vi "DialogCreateMethod.vi"(0 "ClassWriterNative":refnum<class "ClassWriterNative.lvclass">, 1 "ClassItemRefIn":refnum<vi>, 5 "error in (no error)":errorcluster) -> (14 "ClassWriterNative":refnum<class "ClassWriterNative.lvclass">, 15 "ClassItemRefOut":refnum<vi>, 16 "CreateMethodData":T3={"MethodName"="", "RelativeMethodPath"=path "", "MethodDescription"="", "Scope/Visibility"=enum."Use Parent Folder Scope", "MethodTemplateName"="", "IconOut"=[], "RelativeProjectClassPath"="", "OpenViAfterCreation"=FALSE, "DynamicDispatchVi"=FALSE, "ExtraCreateParameters"=variant, "MustOverride"=FALSE, "MustCallParent"=FALSE, "IconDetails"={"IconSize"=enum."1 c-term high", "ImageRows(32)"=32, "ConnectorPaneHeight"=[]}, "AF-Option"=variant, "TemplatePath"=path ""} {"IconOut" format="%x"}, 17 "Cancelled":bool, 19 "error out":errorcluster)   [LabVIEW 2020, in "ClassWriterNative.lvclass"]
uses:
  <resource>/Framework/Providers/Open_GDS/ClassProviders/Provider_LvNativeClass/ClassWriterNative_class/ClassWriterNative.lvclass
  <resource>/Framework/Providers/Open_GDS/ClassProviders/Common/LvIcon_class/GDSLvIcon_ColorControl.ctl
  <resource>/Framework/Providers/Open_GDS/ClassProviders/Provider_BaseClassInterface/CreateMethodData.ctl
  <resource>/Framework/Providers/Open_GDS/ClassProviders/Provider_EndevoGOOP300/GOOP300_SubVIs/GOOP300_MethodScopeType.ctl
  <resource>/Framework/Providers/Open_GDS/ClassProviders/Provider_LvNativeClass/ClassWriterNative_class/IconDetails.ctl
  <resource>/Framework/Providers/Open_GDS/ClassProviders/Provider_LvNativeClass/ClassWriterNative_class/IconSize.ctl
  <resource>/Framework/Providers/Open_GDS/ClassProviders/Common/LvClass_class/GDSLvClass_PlugIn.ctl
  <resource>/Framework/Providers/Open_GDS/ClassProviders/Common/LvClass_class/GDSLvClass_PlugInTypes.ctl
  <resource>/Framework/Providers/Open_GDS/ClassProviders/Provider_LvNativeClass/ClassWriterNative_class/MethodInfo.ctl
  <resource>/Framework/Providers/Open_GDS/ClassProviders/Provider_LvNativeClass/ClassWriterNative_class/MethodType.ctl
  <resource>/Framework/Providers/Open_GDS/ClassProviders/Provider_LvNativeClass/ClassWriterNative_class/MethodInfo_Option.ctl
  <vilib>/Utility/miscctls.llb/LVPoint32TypeDef.ctl
  <vilib>/picture/picture.llb/imagedata.ctl
  <resource>/Framework/Providers/Open_GDS/ClassProviders/Provider_BaseClassInterface/ClassWriter_class/TemplateSettings.ctl
  <vilib>/Utility/miscctls.llb/LVRectTypeDef.ctl
  <resource>/Framework/Providers/Open_GDS/ClassProviders/Provider_EndevoGOOP400/EndevoG4ProviderName.ctl
  <vilib>/event_ctls.llb/lveventtype.ctl
  <resource>/Framework/Providers/Open_GDS/ClassProviders/Common/IconEditor/private/GDSIconEditor_IconDialog_Input.vi
  <resource>/Framework/Providers/Open_GDS/ClassProviders/Common/LvIcon_class/subvis/GDSLvIcon_TextDataType.ctl
  <resource>/Framework/Providers/Open_GDS/ClassProviders/Common/LvIcon_class/GDSLvIcon_WordCompressionType.ctl
  <resource>/Framework/Providers/Open_GDS/ClassProviders/Common/LvIcon_class/GDSLvIcon_TextAlignment.ctl
  <vilib>/Utility/miscctls.llb/LVPositionTypeDef.ctl
  <vilib>/Utility/miscctls.llb/LVPointTypeDef.ctl
  d442fafc-3c31-4c15-9ed3-3a3a20f58e2f.vi
  76481c0e-b793-4274-9995-712af1244245.vi
  <vilib>/Utility/config.llb/Read Key (String).vi
  <vilib>/regexp/Match Regular Expression.xnode
  <resource>/Framework/Providers/Open_GDS/ClassProviders/Provider_BaseClassInterface/ClassWriter_class/ClassWriter.lvclass
  <vilib>/Utility/lvfile.llb/NI_FileType.lvlib
  <vilib>/Utility/config.llb/NI_LVConfig.lvlib
panel:
  in  "PropertyNodeMethodNaming":enum16{"Read/Write Naming", "Get/Set Naming"}(ring) caption="Naming"
  out "MethodTemplateImage":picture
  out "_MethodsLocationOverrideInfo":string=" \n\n" caption="The method's location is controlled by\nthe method you override."
  in  "ClearIcon":bool
  in  "_AddFolder":bool
  in  "Filter":string
  in  ".vim":bool
  out "ProductPicture":picture
  out "_IconPreview":picture caption="Icon Preview"
  in  "_AddMessageClass":bool
  in  "_MethodIcons":bool
  in  "_TextAlignment":u16(ring) caption="Text Alignment" items=["Center", "Left", "Right"]
  in  "_IconSize":u16(ring) caption="Icon Size" items=["Full", "1 c-term high", "2 c-term high", "3 c-term high"]
  in  "_MustCallParent":bool caption="Must Call Parent"
  in  "_MustOverride":bool caption="Must Override"
  out "_VisibilityAndLlocationGrouping":string caption="Visibility and location"
  out "_IconGrouping":string caption="Icon"
  in  "_MethodSignature":u16(ring) caption="Method signature" items=["No signature", "-", "Add signature"]
  in  "_ShowContextHelp":bool
  in  "Help":bool
  in  "_CreateOpenClass":bool
  in  "_MethodIconName":string caption="Body Text"
  in  "_BodyBk":T1 caption="Body Background"
  in  "_BodyText":T1 caption="Body text"
  in  "_FontCompression":enum16{"Auto", "On", "Off"}(ring) caption="Font Compression"
  in  "_CapitalOnly":bool=TRUE caption="Force Capital Letters"
  out "_DubMethodName":string caption="This method already exists in the class"
  out "_Loading":string caption="Loading..."
  in  "_OverrideMethods":i32(listbox) caption="Override Methods"
  in  "_MethodType":T2(radio) caption="Method Type"
  in  "_Property":string[](tree) caption="Data Fields/Attributes"
  in  "_DynamicDispatch":bool caption="Dynamic Dispatch"
  in  "_Visibility":T7(radio) caption="Visibility"
  in  "_MethodLocation":i32(listbox) caption="Method Location"
  in  "_MethodName":string caption="Property Name"
  in  "_Cancel":bool
  in  "_CreateMethod":bool
  in  "_MethodDescription":string caption="Method description"
  in  "_Method":i32[](listbox) caption="Method Template"
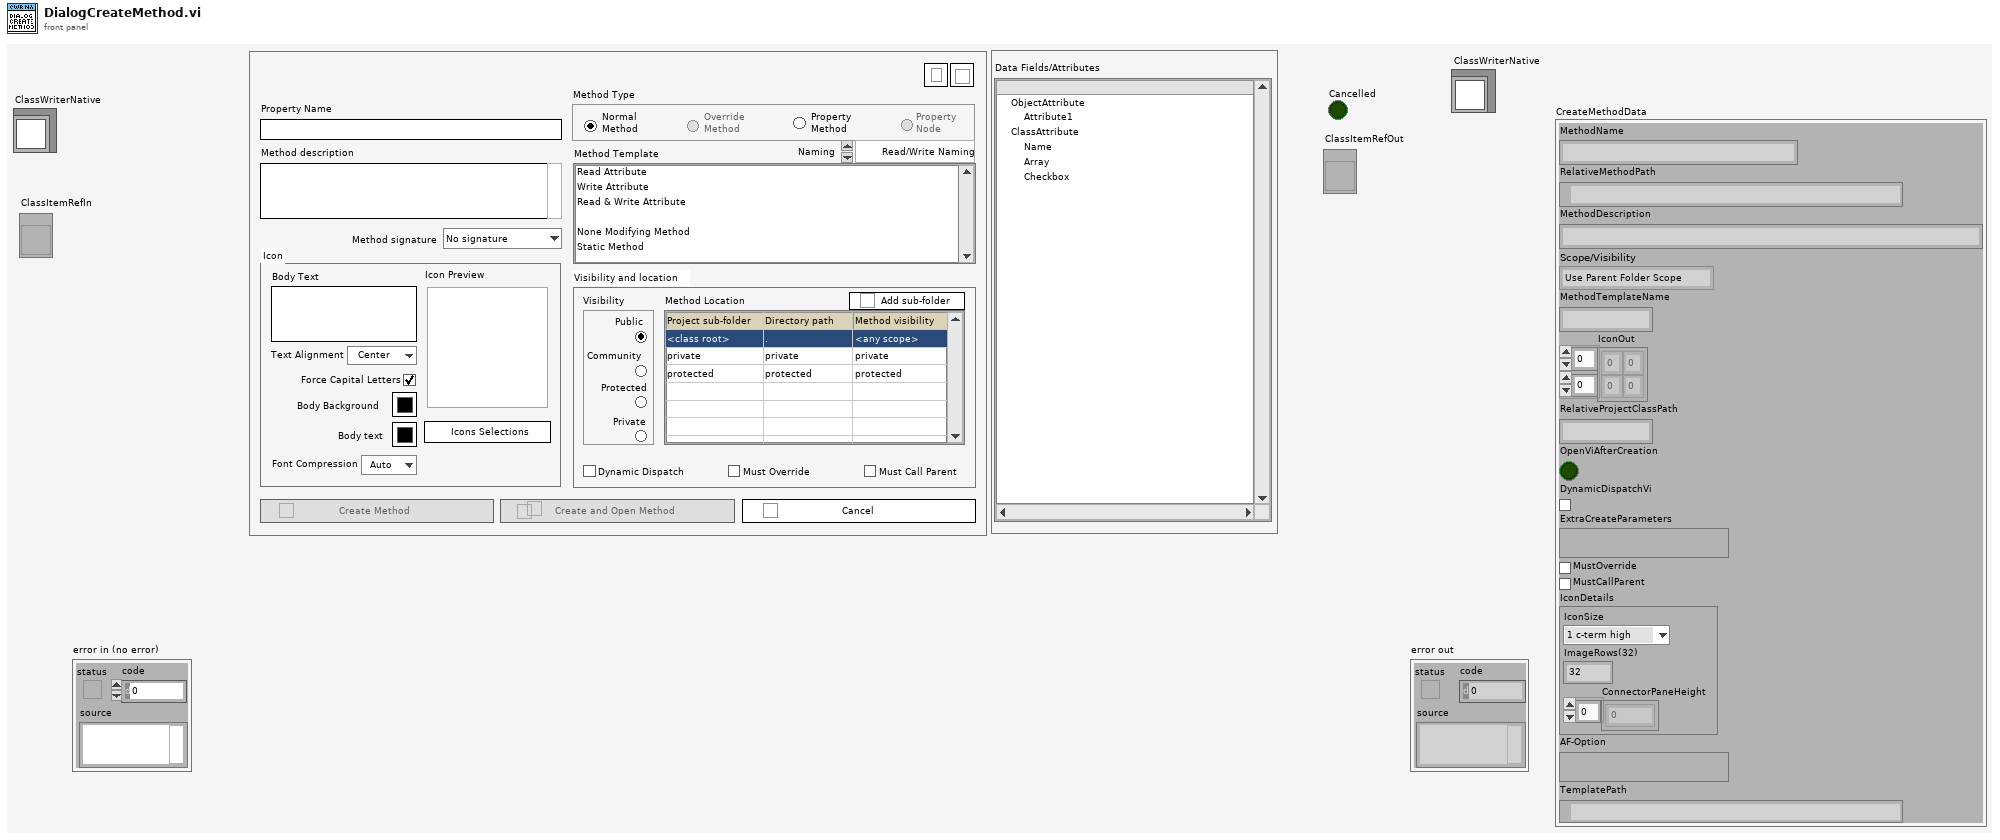
[diagram p1: front panel]
types:
  T1 = typedef "GDSLvIcon_ColorControl.ctl" = cluster{"Decal":bool, "Color":u32}
  T2 = enum32{"Normal Method", "Override Method", "Property Method", "Property Node"}
  T3 = typedef "ClassWriter.lvclass/CreateMethodData.ctl" = cluster{"MethodName":string, "RelativeMethodPath":path, "MethodDescription":string, "Scope/Visibility":T4, "MethodTemplateName":string, "IconOut":u8[][], "RelativeProjectClassPath":string, "OpenViAfterCreation":bool, "DynamicDispatchVi":bool, "ExtraCreateParameters":variant, "MustOverride":bool, "MustCallParent":bool, "IconDetails":T5, "AF-Option":variant, "TemplatePath":path}
  T4 = typedef "GOOP300_MethodScopeType.ctl" = enum16{"Use Parent Folder Scope", "Public", "Protected", "Private", "Community"}
  T5 = typedef "ClassWriterNative.lvclass/IconDetails.ctl" = cluster{"IconSize":T6, "ImageRows(32)":i32, "ConnectorPaneHeight":i32[]}
  T6 = typedef "ClassWriterNative.lvclass/IconSize.ctl" = enum16{"Full", "1 c-term high", "2 c-term high", "3 c-term high"}
  T7 = enum32{"Public", "Community", "Protected", "Private"}
  T8 = cluster{"Font Name":string, "Size":u16, "Bold":bool, "Italic":bool, "Underline":bool, "Strikeout":bool, "Color":u32}
  T9 = cluster{"AttributeNames":string[], "PropertyNode":bool, "FolderNames":string[]}
  T10 = typedef "GDSLvClass_PlugIn.ctl" = cluster{"Type":T11, "ID":string, "Version":string, "Path":path, "Name":string, "Data":variant}
  T11 = typedef "GDSLvClass_PlugInTypes.ctl" = enum16{"DesignPattern", "MethodTypes"}
  T12 = typedef "ClassWriterNative.lvclass/MethodInfo.ctl" = cluster{"Type":T13, "Name":string, "Path":path, "ExtraName":string, "Data":variant, "DynamicDispatch":T14}
  T13 = typedef "ClassWriterNative.lvclass/MethodType.ctl" = enum16{"Normal", "MethodPlugIn", "DesignPattern", "AF-Method"}
  T14 = typedef "ClassWriterNative.lvclass/MethodInfo_Option.ctl" = enum16{"Default", "OnAtStart", "OffAtStart", "AlwaysOn", "AlwaysOff"}
  T15 = typedef "LVPoint32TypeDef.ctl" = cluster{"Horizontal":i32, "Vertical":i32}
  T16 = typedef "imagedata.ctl" = cluster{"image type":i32, "image depth":i32, "image":u8[], "mask":u8[], "colors":u32[], "Rectangle":cluster{"left":i16, "top":i16, "right":i16, "bottom":i16}}
  T17 = typedef "ClassWriter.lvclass/TemplateSettings.ctl" = cluster{"CommonClassTemplate":bool, "DynamicDispatch":enum8{"False", "True", "Mixed"}, "MustOverride":enum8{"False", "True", "Mixed"}, "MustCallParent":enum8{"False", "True", "Mixed"}, "OnlyNormalMethod":bool, "OnlyPublic":bool}
  T18 = cluster{"Cancel":bool, "FolderNames":string[], "FolderPath":path[], "FolderType":enum32{"invalid scope", "public", "private", "protected", "community"}[], "ClassName":string, "ColorProtected":u32, "ColorPrivate":u32, "ColorPublic":u32, "Frame":u32, "Frame thickness":i32, "HeaderIcon":u8[][], "BodyIconHeight":i32, "BodyIconWidth":i32, "RelFolderPath":path[], "MethodIcon":u8[][], "OverRideLookUpDone":bool, "PropertyLookUpDone":bool, "AllOverrideMethods":path[], "ClassVIs":string[], "Open":bool, "OverrideScope":enum32{"invalid scope", "public", "private", "protected", "community"}[], "Signatures":cluster{"SignatureName":string[], "SignatureText":string[], "Current":i32}, "DesignPatterns":T10[], "NormalMethods":T12[], "OverrideMethods":T12[], "PropertyMethods":T12[], "MethodNames":string[], "ConnectorPaneHeight":i32[], "IconDetails":T5, "Offset":cluster{"X":i32, "Y":i32}, "OldOffset":cluster{"X":i32, "Y":i32}, "TextBounds":cluster{"FirstRow":i32, "FirstColumn":i32, "LastRow":i32, "LastColumn":i32}, "DraggingText":bool, "StartTextDraggingPos":T15, "Folders":path[], "IconPaths":cluster{i32, "path out":path}[], "Icons":T16[], "IconNames":string[], "DraggingIcon":bool, "StartTextDraggingPos 2":T15, "BgIconOffset":cluster{"X":i32, "Y":i32}, "Offset 2":cluster{"X":i32, "Y":i32}, "OldOffset 2":cluster{"X":i32, "Y":i32}, "CurrentIcon":cluster{"BgIcon":u8[][], "BgIconOffset":cluster{"X":i32, "Y":i32}, "BgIconMask":u8[], "ColorsOkayforiconToBeOnTopOf":u8[]}, "BgIconMask":u8[], "BodyIcon":u8[][], "BgIcon":u8[][], "HeaderBkColor":u32, "IconOut":u8[][], "IconSelected":i32, "IconDropped":i32, "Moving":bool, "IconPos":cluster{"left":i16, "top":i16, "right":i16, "bottom":i16}[], "BodyIconOut":u8[][], "AF":bool, "ActorVersion":string, "AF-MethodNames":string[], "AF-Methods":cluster{T12[]}[], "AF-Method":i32, "PropertyNodeMethods":T12[], "MethodLocation":string[][], "MethodCaptionName":string, "IsAPropertyDefinitionVI":bool[], "TemplateSettings":T17, "OverrideMethod":path, "Interface":bool, "RowStart(0)":i32, "ImageRows(32)":i32, "MethodVIs":path[], "MethodItemNames":string[], "OverrideMethodsNames":string[], "OverrideMethodsIdx":i32[], "Methods.DynamicDispatch":T14[], "Splitter0px":bool}
  T19 = enum8{"Enabled", "Disabled", "Disabled and Grayed Out"}
  T20 = enum16{"Full", "1 c-term high", "2 c-term high", "3 c-term high", "Off"}
  T21 = typedef "EndevoG4ProviderName.ctl" = enum16{"EndevoGOOP400"}
  T22 = enum32{"invalid scope", "public", "private", "protected", "community"}
  T23 = typedef "LVRectTypeDef.ctl" = cluster{"Left":i16, "Top":i16, "Right":i16, "Bottom":i16}
  T24 = typedef "lveventtype.ctl" = enum32{"Null", "Timeout", "Annotation Menu Selection", "Annotation Menu Selection?", "App Instance Close", "App Instance Close?", "Autoscale Range Change", "Bookmark Info Change", "Cell Edit", "Cell Edit?", "Cursor Grab", "Cursor Grab?", "Cursor Menu Selection", "Cursor Menu Selection?", "Cursor Move", "Cursor Release", "Data Change", "Direction Change", "Display State Change", "Drag Ended", "Drag Enter", "Drag Leave", "Drag Over", "Drag Source Update", "Drag Starting", "Drag Starting?", "Drop", "Exec State Change", "Key Down", "Key Down?", "Key Repeat", "Key Repeat?", "Key Up", "Listbox Double Click", "Menu Activation?", "Menu Selection (App)", "Menu Selection? (App)", "Menu Selection (User)", "Mouse Down", "Mouse Down?", "Mouse Enter", "Mouse Leave", "Mouse Move", "Mouse Up", "Mouse Wheel", "NI Security User Change (App)", "Pane Size", "Panel Close", "Panel Close?", "Panel Resize", "Plot Attribute Change", "Scale Range Change", "Shortcut Menu Activation?", "Shortcut Menu Selection (App)", "Shortcut Menu Selection? (App)", "Shortcut Menu Selection (User)", "Tree Double Click", "Tree Drag", "Tree Drag?", "Tree Drop", "Tree Drop?", "Tree Item Close", "Tree Item Close?", "Tree Item Open", "Tree Item Open?", "User Event", "Value Change"}
  T25 = typedef "GDSIconEditor_IconDialog_Input.vi" = cluster{"HeaderIcon":u8[][], "RowStart(0)":i32, "ImageRows(32)":i32, "FrameThickness(1)":u32, "FrameColor":u32, "IconTextDataType":T26, "BodyTextColor":u32, "BodyBackgroundColor":u32, "BodyIconHeight":i32, "BodyIconWidth":i32, "HeaderBackgroundColor":u32, "BodyIcon":u8[][], "Offset":cluster{"X":i32, "Y":i32}, "CurrentIcon":cluster{"BgIcon":u8[][], "BgIconOffset":cluster{"X":i32, "Y":i32}, "BgIconMask":u8[], "ColorsOkayforiconToBeOnTopOf":u8[]}}
  T26 = typedef "GDSLvIcon_TextDataType.ctl" = cluster{"Text":string, "Allow Only Capital Chars":bool, "Compression":T27, "Alignment":T28}
  T27 = typedef "GDSLvIcon_WordCompressionType.ctl" = enum16{"Auto", "On", "Off"}
  T28 = typedef "GDSLvIcon_TextAlignment.ctl" = enum16{"Center", "Left", "Right"}
  T29 = cluster{"BgIcon":u8[][], "BgIconOffset":cluster{"X":i32, "Y":i32}, "BgIconMask":u8[], "ColorsOkayforiconToBeOnTopOf":u8[]}
  T30 = typedef "LVPositionTypeDef.ctl" = cluster{"Left":i32, "Top":i32}
  T31 = typedef "LVPointTypeDef.ctl" = cluster{"Horizontal":i16, "Vertical":i16}
  T32 = typedef "GOOP400_Options.ctl" = cluster{"FlatFolderStructure":bool}
  T33 = enum32{"invalid scope", "public", "private", "protected", "community"}[]
  T34 = typedef "BaseProvider_IniFileSettings.ctl" = cluster{"ClassFolderSuffix":string, "InterfaceFolderSuffix":string, "InterfaceIcon":string, "FileNamingOption":T35, "DynamicDispatchStartValue":bool, "UseGetSetForPropertyNodeMethods":bool}
  T35 = typedef "BaseProvider_FileNamingOption.ctl" = enum16{"CamelCase", "Space", "Underscore"}
  T36 = cluster{"Major":u16, "Minor":u16, "Fix":u16, "Build":u16}
  T37 = typedef "AF_ClassType.ctl" = enum16{"NA", "Actor", "Message"}
  T38 = typedef "GDSLvClass_IconSettingsType.ctl" = cluster{"Frame":u32, "Frame thickness":u8, "Header Background":u32, "Header Text":u32, "ColorPublic":u32, "ColorProtected":u32, "ColorPrivate":u32, "Body Text":u32, "ClassBodyIcon":string}
  T39 = cluster{"SignatureName":string[], "SignatureText":string[], "Current":i32}
  T40 = typedef "eventvkey.ctl" = enum16{"ASCII", "Enter", "Return", "Shift", "Ctrl", "Alt", "Cmd", "Opt", "Caps", "NumLock", "Clear", "Break", "Up", "Down", "Left", "Right", "Insert", "Delete", "Home", "End", "PageUp", "PageDown", "Escape", "Help", "Pause", "ScrollLock", "F1", "F2", "F3", "F4", "F5", "F6", "F7", "F8", "F9", "F10", "F11", "F12", "F13", "F14", "F15", "F16", "F17", "F18", "F19", "F20", "F21", "F22", "F23", "F24", "Play", "VolumeUp", "VolumeDown", "Mute", "Two Byte Char"}
  T41 = typedef "LVMouseTypeDef.ctl" = cluster{"Mouse Position":cluster{"X":i32, "Y":i32}, "Mouse Modifiers":cluster{"Button Down":bool, "Shift Mod":bool, "Menu Mod":bool, "Option Mod":bool}}
  T42 = cluster{"FirstRow":i32, "FirstColumn":i32, "LastRow":i32, "LastColumn":i32}
  T43 = typedef "ColorControl.ctl" = cluster{"Decal":bool, "Color":u32}
  T44 = typedef "LVBoundsTypeDef.ctl" = cluster{"Width":u32, "Height":u32}
  T45 = cluster{"left":i16, "top":i16, "right":i16, "bottom":i16}
  T46 = typedef "NI_LVConfig.lvlib/Config Data RefNum.ctl" = refnum<k1>
  T47 = cluster{"PlugInName":string, "MethodSelected":string}
  T48 = cluster{"SignatureName":string[], "SignatureText":string[], i32}
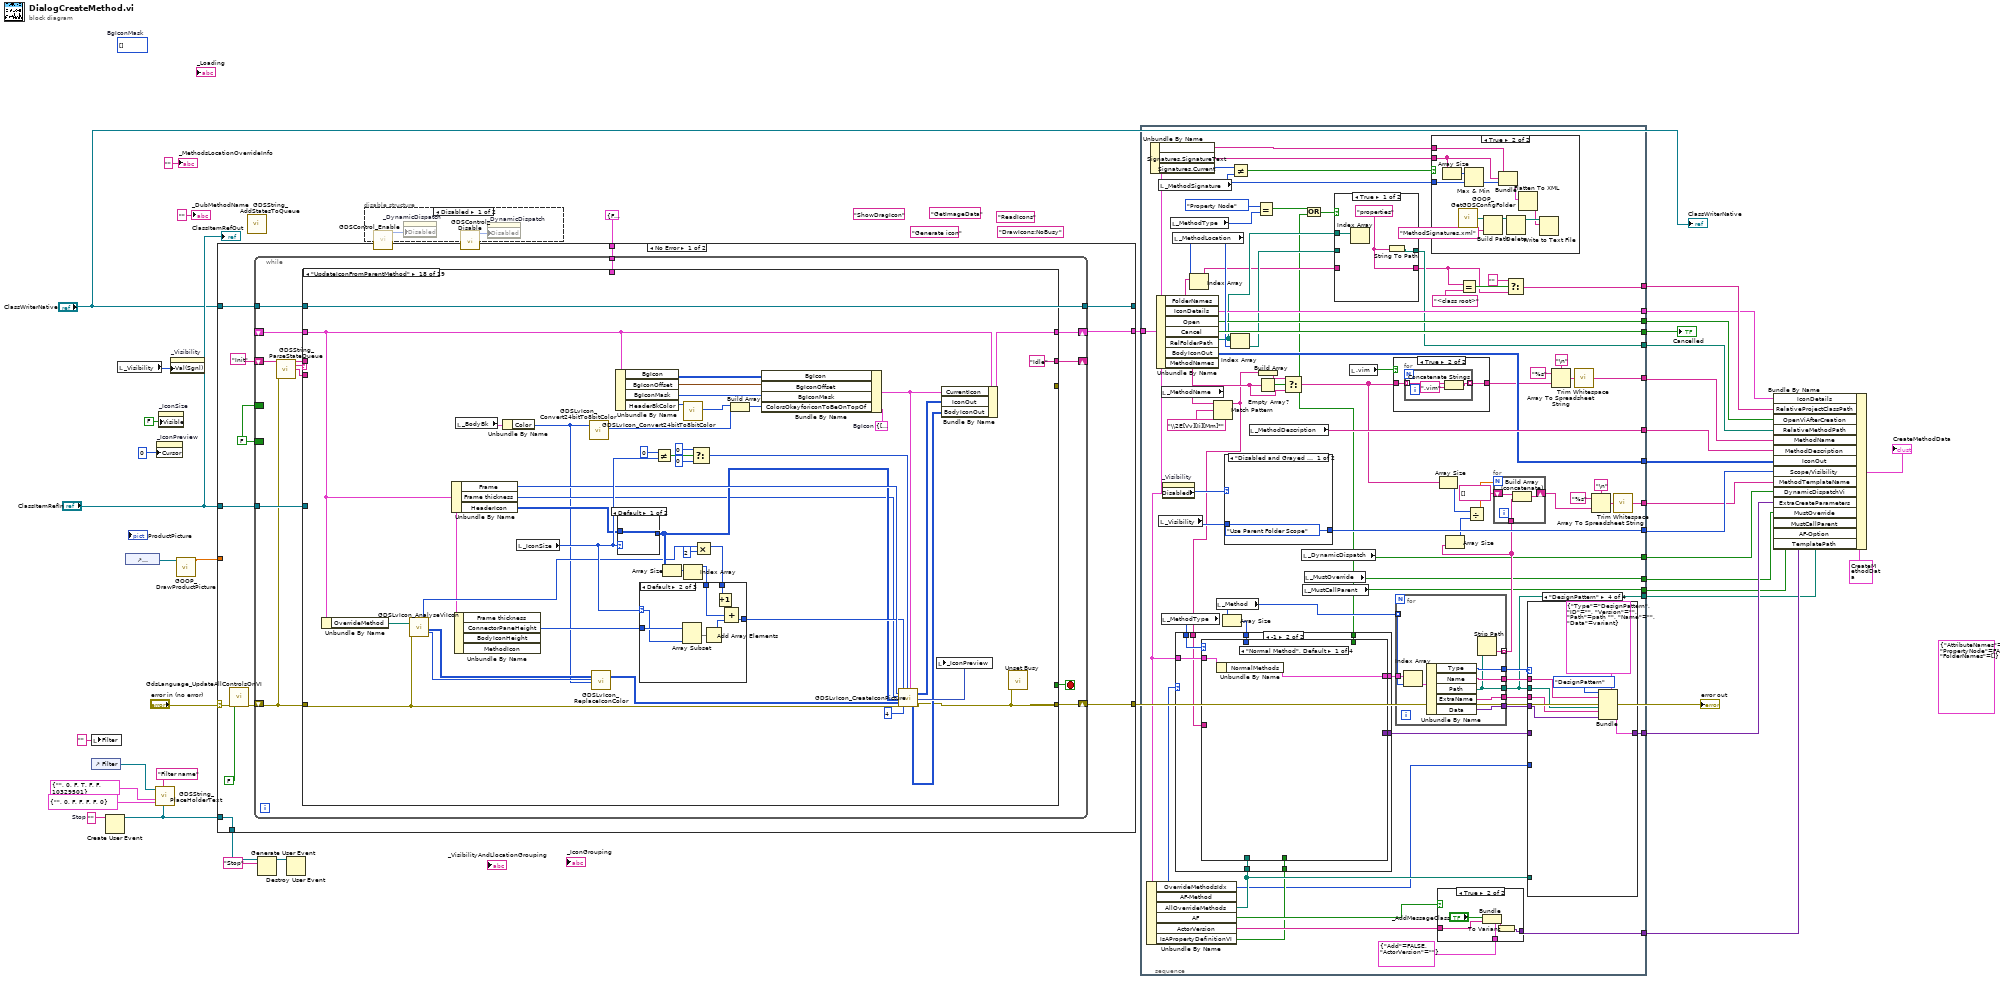
[diagram p0: block diagram]
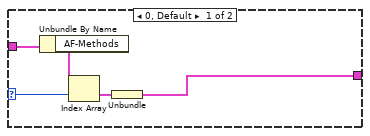
[diagram p5: hidden frame]
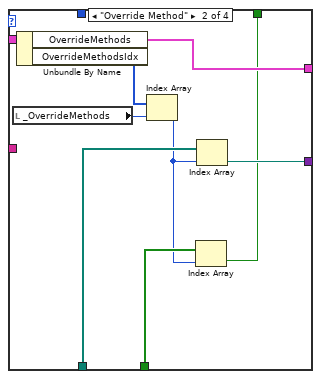
[diagram p6: hidden frame]
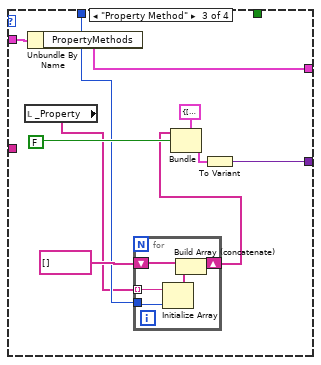
[diagram p7: hidden frame]
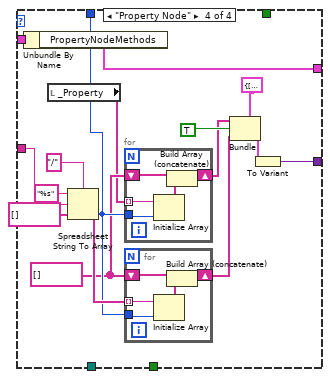
[diagram p8: hidden frame]
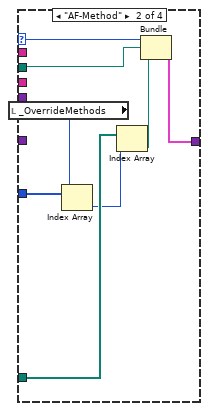
[diagram p11: hidden frame]
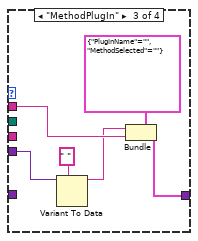
[diagram p12: hidden frame]
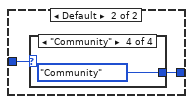
[diagram p14: hidden frame]
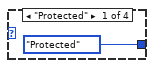
[diagram p15: hidden frame]
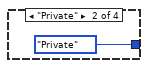
[diagram p16: hidden frame]
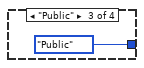
[diagram p17: hidden frame]
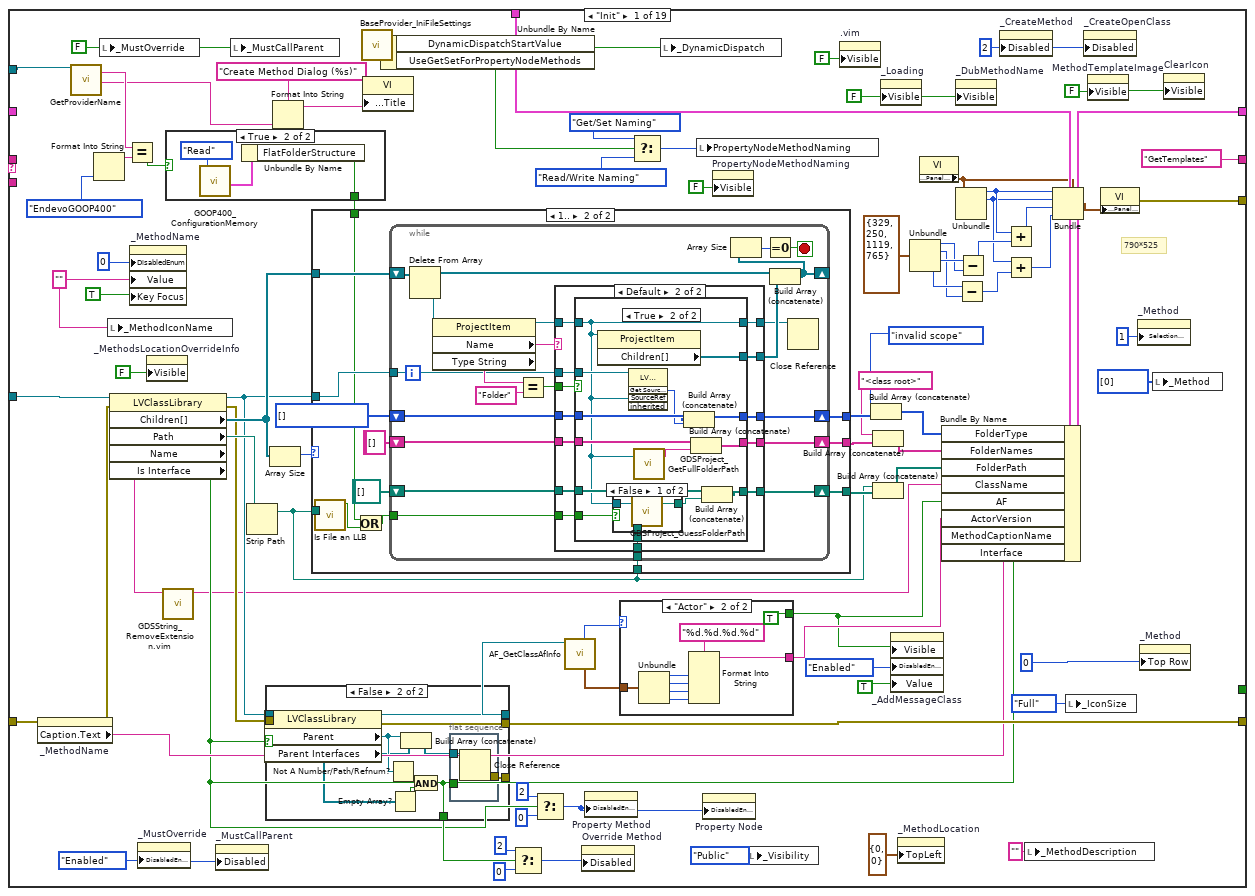
[diagram p18: hidden frame]
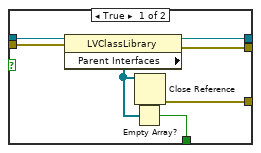
[diagram p20: hidden frame]
diagram:
  (unwired) "Generate icon"
  (unwired) "ShowDragIcon" ("t")
  (unwired) "GetImageData" ("y")
  (unwired) "DrawIcons:NoBusy" ("y")
  (unwired) "ReadIcons"
  w8 = ""  # Stop
  (unwired) T9 {"AttributeNames"=[], "PropertyNode"=FALSE, "FolderNames"=[]} ("cluster")
  (unwired) u8[] []  # BgIconMask
  n1 = control-ref of="Filter"() -> (w2:refnum<vi>)
  n2 = local write "Filter"("" ("Filter")) -> ()
  n3 = Create User Event(user event datatype=w8) -> (user event=w4:refnum<user-event>)  [unwired: 1 in, 1 out]
  n4 = local read "_Visibility"() -> (w11:T7)
  n5 = control-ref of="ProductPicture"() -> (w16:refnum<vi>)
  n6 = call <resource>:"GDSString_PlaceHolderText.vi"("BooleanUserEventToStopPlaceHolderVI"=w4, "PlaceholderText"="Filter name" ("InterfaceFilter"), "PlaceholderTextFont(Grey,Italic)"=T8 {"Font Name"="", "Size"=0, "Bold"=FALSE, "Italic"=TRUE, "Underline"=FALSE, "Strikeout"=FALSE, "Color"=10329501}, "NormalTextFont(Black)"=T8 {"Font Name"="", "Size"=0, "Bold"=FALSE, "Italic"=FALSE, "Underline"=FALSE, "Strikeout"=FALSE, "Color"=0}, "PlaceholderStringRef"=w2) -> ()  [unwired: 6 in, 1 out]
  n7 = property on="_IconPreview" class="Pict"("Cursor"=0) -> ()  [unwired: 2 in, 2 out]
  n8 = property on="_IconSize" class="Ring (strict)"("Visible"=FALSE) -> ()  [unwired: 2 in, 2 out]
  n9 = property on="_Visibility" class="RadioBtnsControl (strict)"("Val(Sgnl)"=w11) -> ()  [unwired: 2 in, 2 out]
  n10 = call <resource>:"GOOP_DrawProductPicture.vi"("ProductPictureControl"=w16) -> ("Zoom Factor"=w15:sgl)  [unwired: 10 in]
  n11 = case shown="No Error" "error in (no error)" {
    selector: "error in (no error)" -> [w47 w2528]
    tunnel: "ClassWriterNative" -> [w51 w2527]
    tunnel: [w53 w2528] -> w27
    tunnel: [w52 w2527] -> _
    tunnel: T18 {"Cancel"=FALSE, "FolderNames"=[], "FolderPath"=[], "FolderType"=[], "ClassName"="", "ColorProtected"=16777215, "ColorPrivate"=16777215, "ColorPublic"=16121600, "Frame"=0, "Frame thickness"=3, "HeaderIcon"=[], "BodyIconHeight"=0, "BodyIconWidth"=0, "RelFolderPath"=[], "MethodIcon"=[], "OverRideLookUpDone"=FALSE, "PropertyLookUpDone"=FALSE, "AllOverrideMethods"=[], "ClassVIs"=[], "Open"=FALSE, "OverrideScope"=[], "Signatures"={"SignatureName"=[], "SignatureText"=[], "Current"=-1}, "DesignPatterns"=[], "NormalMethods"=[], "OverrideMethods"=[], "PropertyMethods"=[], "MethodNames"=[], "ConnectorPaneHeight"=[], "IconDetails"={"IconSize"=enum."Full", "ImageRows(32)"=0, "ConnectorPaneHeight"=[]}, "Offset"={"X"=0, "Y"=0}, "OldOffset"={"X"=0, "Y"=0}, "TextBounds"={"FirstRow"=2, "FirstColumn"=1, "LastRow"=6, "LastColumn"=27}, "DraggingText"=FALSE, "StartTextDraggingPos"={"Horizontal"=0, "Vertical"=0}, "Folders"=[], "IconPaths"=[], "Icons"=[], "IconNames"=[], "DraggingIcon"=FALSE, "StartTextDraggingPos 2"={"Horizontal"=0, "Vertical"=0}, "BgIconOffset"={"X"=0, "Y"=0}, "Offset 2"={"X"=0, "Y"=0}, "OldOffset 2"={"X"=0, "Y"=0}, "CurrentIcon"={"BgIcon"=[], "BgIconOffset"={"X"=0, "Y"=0}, "BgIconMask"=[], "ColorsOkayforiconToBeOnTopOf"=[]}, "BgIconMask"=[], "BodyIcon"=[[0, 0, 0, 0, 0, 0, 0, 0, 0, 0, 255, 255, 0, 0, 255, 0, 0, 0, 255, 0, 0, 0, 0, 0, 0, 0, 0, 0, 0, 0], [0, 0, 0, 0, 0, 0, 0, 0, 0, 255, 0, 0, 255, 0, 255, 0, 0, 0, 255, 0, 0, 0, 0, 0, 0, 0, 0, 0, 0, 0], [0, 0, 0, 0, 0, 0, 0, 0, 0, 255, 255, 255, 255, 0, 255, 0, 0, 0, 255, 0, 0, 0, 0, 0, 0, 0, 0, 0, 0, 0], [0, 0, 0, 0, 0, 0, 0, 0, 0, 255, 0, 0, 255, 0, 255, 0, 0, 0, 255, 0, 0, 0, 0, 0, 0, 0, 0, 0, 0, 0], [0, 0, 0, 0, 0, 0, 0, 0, 0, 255, 0, 0, 255, 0, 255, 255, 255, 0, 255, 255, 255, 0, 0, 0, 0, 0, 0, 0, 0, 0], [0, 0, 255, 0, 0, 0, 255, 0, 0, 255, 255, 0, 0, 255, 0, 0, 255, 0, 255, 255, 0, 255, 255, 0, 0, 0, 255, 255, 0, 0], [0, 255, 0, 255, 0, 255, 0, 255, 0, 255, 0, 255, 0, 255, 255, 0, 255, 0, 255, 0, 0, 255, 0, 255, 0, 255, 0, 0, 0, 0], [0, 255, 0, 0, 0, 255, 0, 255, 0, 255, 255, 0, 0, 255, 0, 255, 255, 0, 255, 255, 0, 255, 255, 0, 0, 0, 255, 0, 0, 0], [0, 255, 0, 255, 0, 255, 0, 255, 0, 255, 0, 255, 0, 255, 0, 0, 255, 0, 255, 0, 0, 255, 0, 255, 0, 0, 0, 255, 0, 0], [0, 0, 255, 0, 0, 0, 255, 0, 0, 255, 0, 255, 0, 255, 0, 0, 255, 0, 255, 255, 0, 255, 0, 255, 0, 255, 255, 0, 0, 0], [0, 255, 0, 0, 0, 255, 0, 0, 255, 0, 0, 255, 0, 255, 0, 0, 255, 0, 255, 255, 0, 0, 255, 0, 0, 255, 255, 255, 0, 255], [255, 0, 255, 0, 255, 0, 255, 0, 255, 255, 0, 255, 0, 255, 255, 0, 255, 0, 255, 0, 0, 255, 0, 255, 0, 0, 255, 0, 0, 255], [255, 0, 0, 0, 255, 0, 255, 0, 255, 0, 255, 255, 0, 255, 0, 255, 255, 0, 255, 255, 0, 255, 0, 0, 0, 0, 255, 0, 0, 255], [255, 0, 255, 0, 255, 0, 255, 0, 255, 0, 0, 255, 0, 255, 0, 0, 255, 0, 255, 0, 0, 255, 0, 255, 0, 0, 255, 0, 0, 255], [0, 255, 0, 0, 0, 255, 0, 0, 255, 0, 0, 255, 0, 255, 0, 0, 255, 0, 255, 255, 0, 0, 255, 0, 0, 0, 255, 0, 0, 255], [0, 0, 0, 0, 0, 0, 0, 0, 0, 0, 0, 0, 0, 0, 255, 0, 0, 0, 0, 0, 0, 0, 0, 0, 0, 0, 0, 0, 0, 0], [0, 0, 0, 0, 0, 0, 0, 0, 0, 0, 0, 0, 0, 255, 0, 0, 0, 0, 0, 0, 0, 0, 0, 0, 0, 0, 0, 0, 0, 0], [0, 0, 0, 0, 0, 0, 0, 0, 0, 0, 0, 0, 0, 255, 255, 0, 0, 0, 0, 0, 0, 0, 0, 0, 0, 0, 0, 0, 0, 0], [0, 0, 0, 0, 0, 0, 0, 0, 0, 0, 0, 0, 0, 255, 0, 255, 0, 0, 0, 0, 0, 0, 0, 0, 0, 0, 0, 0, 0, 0], [0, 0, 0, 0, 0, 0, 0, 0, 0, 0, 0, 0, 0, 0, 255, 0, 0, 0, 0, 0, 0, 0, 0, 0, 0, 0, 0, 0, 0, 0], [0, 0, 0, 0, 0, 0, 0, 0, 0, 0, 0, 0, 0, 0, 0, 0, 0, 0, 0, 0, 0, 0, 0, 0, 0, 0, 0, 0, 0, 0], [0, 0, 0, 0, 0, 0, 0, 0, 0, 0, 0, 0, 0, 0, 0, 0, 0, 0, 0, 0, 0, 0, 0, 0, 0, 0, 0, 0, 0, 0]], "BgIcon"=[], "HeaderBkColor"=0, "IconOut"=[], "IconSelected"=0, "IconDropped"=-1, "Moving"=FALSE, "IconPos"=[], "BodyIconOut"=[], "AF"=TRUE, "ActorVersion"="", "AF-MethodNames"=[], "AF-Methods"=[], "AF-Method"=-1, "PropertyNodeMethods"=[], "MethodLocation"=[], "MethodCaptionName"=" ", "IsAPropertyDefinitionVI"=[], "TemplateSettings"={"CommonClassTemplate"=FALSE, "DynamicDispatch"=enum."False", "MustOverride"=enum."False", "MustCallParent"=enum."False", "OnlyNormalMethod"=FALSE, "OnlyPublic"=FALSE}, "OverrideMethod"=path "", "Interface"=TRUE, "RowStart(0)"=0, "ImageRows(32)"=32, "MethodVIs"=[], "MethodItemNames"=[], "OverrideMethodsNames"=[], "OverrideMethodsIdx"=[], "Methods.DynamicDispatch"=[], "Splitter0px"=FALSE} ("output cluster") -> [w50 _]
    tunnel: "ClassItemRefIn" -> [w49 _]
    tunnel: [w48 _] -> w39
    tunnel: w15 -> [_ _]
    tunnel: [w42 w2526] -> w5
    tunnel: w4 -> [w42 w2526]
    frame No Error {
      w43 = FALSE
      n12 = call <resource>:"GdsLanguage_UpdateAllControlsOnVI.vi"("error in (no error)"=w47, "CreateLanguageFile(Use this to create a languageFile)"=FALSE) -> ("error out"=w46:errorcluster)  [unwired: 16 in, 1 out]
      n13 = while {
        shift-right: [w65] -> w53
        shift-left: w46 -> [w56]
        shift-right: [w61] -> _
        shift-left: "Init" -> [w59]
        shift-right: [w66] -> w48
        shift-left: _ -> [w54]
        tunnel: w51 -> [w64]
        tunnel: [w64] -> w52
        tunnel: w50 -> [w63]
        tunnel: w49 -> [w62]
        border: w43 -> [_]
        border: w43 -> [_]
        stop <- w60 stop-if-true
        n14 = call <resource>:"GDSString_ParseStateQueue.vi"("State Queue"=w59, "Error In (no error)"=w56) -> ("Remaining States"=w57:string, "Current State"=w55:string, "Arguments"=w58:string)  [unwired: 9 in, 2 out]
        n15 = case shown="\"UpdateIconFromParentMethod\"" w55 {
          tunnel: w54 -> [_ w259 w342 w377 w396 w469 w502 w1663 w1741 w1787 w1798 w2111 w2156 w2177 w2196 w2300 w2414 w2467 w2521]
          tunnel: [w151 w293 w341 w376 w430 w466 w514 w1663 w1741 w1788 w1836 w2110 w2155 w2176 w2232 w2303 w2416 w2477 w2524] -> w66
          tunnel: w56 -> [w92 w290 w346 w370 w431 w476 w499 w1688 w1764 w1785 w1835 w2116 w2159 w2174 w2239 w2305 w2419 w2471 w2522]
          tunnel: [w98 w264 w346 w369 w390 w476 w500 w1688 w1764 w1785 w1834 w2109 w2150 w2174 w2240 w2305 w2418 w2463 w2522] -> w65
          tunnel: w64 -> [w114 w291 _ _ _ _ w498 _ _ _ _ _ w2152 _ _ _ _ _ _]
          tunnel: ["GetTemplates" w294 w337 "GetClassColors" "UpdateMethodSignatures" "UpdateIcon" w515 w1689 w1747 "Generate icon" "Exit" "Idle" "UpdateIcon" w2188 w2244 "Idle" "Idle" ("item tag") "Idle" ("item tag") "Exit"] -> w61
          tunnel: w63 -> [w149 _ _ _ _ _ _ _ _ _ _ _ _ _ _ _ _ _ _]
          tunnel: w62 -> [w150 w288 w350 w372 w400 _ w497 _ _ _ _ w2115 w2158 _ _ w2314 _ _ _]
          tunnel: [w86 _ _ _ _ _ _ _ _ _ _ _ _ _ _ _ _ _ _] -> _
          tunnel: [_ _ _ _ _ _ _ _ _ _ _ _ _ _ _ _ _ _ TRUE ("Cancel")] -> w60
          tunnel: w58 -> [_ _ _ _ _ _ _ _ _ _ _ _ _ _ _ _ _ _ _]
          tunnel: w57 -> [_ _ w336 _ _ _ _ w1689 w1747 _ _ _ _ w2188 _ _ _ _ _]
          frame "Init" {
            w78 = FALSE ("Visible")
            w89 = FALSE ("Dynamic dispatch")
            w109 = T19."Enabled" ("Disabled")
            w125 = FALSE ("Visible")
            w117 = u8 2 ("Disabled")
            w118 = "" ("Method Name")
            # "790*525"
            n16 = property on="_MethodName" class="Str"(error in=w92) -> (error out=w91:errorcluster, "Caption.Text"=w90:string)  [unwired: 1 in, 1 out]
            n17 = call-dynamic "GetProviderName.vi"("ClassWriterNative in"=w114) -> ("ProviderName"=w81:string, "TranslatedProviderName"=w79:string)  [unwired: 14 in, 3 out]
            n18 = Format Into String(EndevoG4ProviderName."EndevoGOOP400" ("ProviderName")) -> (resulting string=w105:string)  [unwired: 3 in, 1 out]
            n19 = local write "_MustOverride"(w89) -> ()
            n20 = local write "_MethodIconName"(w118) -> ()
            n21 = property class="LVClassLibrary"(reference=w150, error in=w91) -> (reference out=w124:refnum<vi>, error out=w123:errorcluster, "Children[]"=w147:refnum<vi>[], "Path"=w138:path, "Name"=w68:string, "Is Interface"=w83:bool)
            n22 = Equal?(x=w81, y=w105) -> (x = y?=w75:bool)
            n23 = property on="_MethodName" class="Str"("DisabledEnum"=u8 0 ("Disabled"), "Value"=w118, "Key Focus"=TRUE) -> ()  [unwired: 2 in, 2 out]
            n24 = property on="_MustOverride" class="Bool (strict)"("DisabledEnum"=w109) -> ()  [unwired: 2 in, 2 out]
            n25 = property on="_MethodsLocationOverrideInfo" class="Str"("Visible"=FALSE) -> ()  [unwired: 2 in, 2 out]
            n26 = call "GDSString_RemoveExtension.vim"("NameWithExtension"=w68) -> ("NameWithoutExtension"=w67:string)  [unwired: 9 in, 1 out]
            n27 = case shown="True" w75 {
              tunnel: [_ w153] -> w74
              frame False {
              }
              frame True {
                n28 = call <resource>:"GOOP400_ConfigurationMemory.vi"("Action"=enum16{"Read", "Load", "Save"}."Read") -> ("OptionsOut"=w154:T32)  [unwired: 17 in, 1 out]
                n29 = Unbundle By Name(w154) -> ("FlatFolderStructure"=w153:bool)
              }
            }
            n30 = property on="_MustCallParent" class="Bool (strict)"("Disabled"=w109) -> ()  [unwired: 2 in, 2 out]
            n31 = local write "_MustCallParent"(w89) -> ()
            n32 = Strip Path(path=w138) -> (stripped path=w110:path)  [unwired: 1 out]
            n33 = case shown="False" w83 {
              tunnel: w124 -> [w162 w173]
              tunnel: w123 -> [w161 w172]
              tunnel: [w159 w171] -> w98
              tunnel: [w158 w170] -> w97
              tunnel: [w157 w163] -> w87
              tunnel: [w156 w169] -> _
              frame True {
                n34 = property class="LVClassLibrary"(reference=w162, error in=w161) -> (reference out=w158:refnum<vi>, error out=w159:errorcluster, "Parent Interfaces"=w160:refnum<vi>[])
                n35 = Empty Array?(array=w160) -> (empty?=w157:bool)
                n36 = Close Reference(reference=w160) -> (error out=w156:errorcluster)  [unwired: 1 in]
              }
              frame False {
                n37 = property class="LVClassLibrary"(reference=w173, error in=w172) -> (reference out=w170:refnum<vi>, error out=w171:errorcluster, "Parent"=w167:refnum<vi>, "Parent Interfaces"=w166:refnum<vi>[])
                n38 = Not A Number/Path/Refnum?(number/path/refnum=w167) -> (NaN/Path/Refnum?=w165:bool)
                n39 = Empty Array?(array=w166) -> (empty?=w164:bool)
                n40 = Build Array (concatenate)(w167, w166) -> (w168:refnum<vi>[])
                n41 = And(x=w165, y=w164) -> (x .and. y?=w163:bool)
                n42 = flat-sequence {
                  tunnel: [w175] -> w169
                  tunnel: w168 -> [w174]
                  tunnel: w163 -> [_]
                  frame #0 {
                    n43 = Close Reference(reference=w174) -> (error out=w175:errorcluster)  [unwired: 1 in]
                  }
                }
              }
            }
            n44 = Array Size(array=w147) -> (size(s)=w146:i32)
            n45 = Format Into String(format string="Create Method Dialog (%s)", w79) -> (resulting string=w116:string)  [unwired: 2 in, 1 out]
            n46 = case shown="1.." w146 {
              tunnel: w147 -> [_ w196]
              tunnel: [_ w194] -> w144
              tunnel: [_ w193] -> w140
              tunnel: [_ w190] -> w142
              tunnel: w124 -> [_ w189]
              tunnel: w110 -> [_ w188]
              tunnel: w110 -> [_ w187]
              tunnel: w74 -> [_ w185]
              frame 0, Default {
              }
              frame 1.. {
                w191 = T33 [] items=["invalid scope", "public", "private", "protected", "community"]
                (unwired) path[] []
                (unwired) string[] []
                n47 = call <vilib>:"Is File an LLB.vi"("path"=w188) -> ("Is LLB?"=w186:bool)  [unwired: 9 in, 1 out]
                n48 = Or(x=w185, y=w186) -> (x .or. y?=w184:bool)
                n49 = while {
                  shift-right: [w199] -> _
                  shift-left: w196 -> [w218]
                  shift-right: [w208] -> w194
                  shift-left: path[] [] -> [w207]
                  shift-right: [w201] -> w193
                  shift-left: string[] [] -> [w204]
                  shift-right: [w202] -> w190
                  shift-left: w191 -> [w203]
                  tunnel: w189 -> [w200]
                  tunnel: w184 -> [w198]
                  tunnel: w187 -> [w197]
                  stop <- w215 stop-if-true
                  n50 = Delete From Array(array=w218) -> (deleted portion=w214:refnum<vi>, array with subset deleted=w217:refnum<vi>[])  [unwired: 2 in]
                  n51 = property class="ProjectItem"(reference=w214) -> (reference out=w210:refnum<vi>, "Name"=w205:string, "Type String"=w213:string)  [unwired: 1 in, 1 out]
                  n52 = Equal?(x=w213, y="Folder") -> (x = y?=w211:bool)
                  n53 = case shown="Default" w205 {
                    tunnel: w211 -> [_ w235]
                    tunnel: w210 -> [w221 w234]
                    tunnel: [_ w233] -> w209
                    tunnel: [w219 w226] -> w201
                    tunnel: [w222 w232] -> w208
                    tunnel: w207 -> [w222 w231]
                    tunnel: [w221 w230] -> w206
                    tunnel: w204 -> [w219 w229]
                    tunnel: w203 -> [w220 w228]
                    tunnel: [w220 w227] -> w202
                    tunnel: w200 -> [_ w225]
                    tunnel: w198 -> [_ w224]
                    tunnel: w197 -> [_ w223]
                    frame "Util", "Utils" {
                    }
                    frame Default {
                      n54 = case shown="True" w235 {
                        tunnel: w234 -> [w238 w243]
                        tunnel: [_ w253] -> w233
                        tunnel: [w236 w252] -> w226
                        tunnel: w231 -> [w239 w250]
                        tunnel: [w239 w251] -> w232
                        tunnel: [w238 w243] -> w230
                        tunnel: w229 -> [w236 w246]
                        tunnel: w228 -> [w237 w248]
                        tunnel: [w237 w247] -> w227
                        tunnel: w225 -> [_ w245]
                        tunnel: w224 -> [_ w241]
                        tunnel: w223 -> [_ w240]
                        frame False {
                        }
                        frame True {
                          n55 = property class="ProjectItem"(reference=w243) -> ("Children[]"=w253:refnum<vi>[])  [unwired: 1 in, 2 out]
                          n56 = case shown="False" w241 {
                            tunnel: [w255 w256] -> w249
                            tunnel: w243 -> [w254 _]
                            tunnel: w240 -> [_ w256]
                            frame False {
                              n57 = call <resource>:"GDSProject_GuessFolderPath.vi"("ProjectItem"=w254) -> ("Path"=w255:path)  [unwired: 15 in, 3 out]
                            }
                            frame True {
                            }
                          }
                          n58 = invoke class="LVClassLibrary" method="Get Source Scope"(reference=w245, "SourceRef"=w243) -> ("GetSourceScope"=w244:T22)  [unwired: 3 in, 4 out]
                          n59 = call <resource>:"GDSProject_GetFullFolderPath.vi"("Folder Item"=w243) -> ("ProjectClassPath"=w242:string)  [unwired: 17 in, 1 out]
                          n60 = Build Array (concatenate)(w248, w244) -> (w247:T33)
                          n61 = Build Array (concatenate)(w246, w242) -> (w252:string[])
                          n62 = Build Array (concatenate)(w250, w249) -> (w251:path[])
                        }
                      }
                    }
                  }
                  n63 = Build Array (concatenate)(w217, w209) -> (w199:refnum<vi>[])
                  n64 = Array Size(array=w199) -> (size(s)=w216:i32)
                  n65 = Equal To 0?(x=w216) -> (x = 0?=w215:bool)
                  n66 = Close Reference(reference=w206) -> ()  [unwired: 1 in, 1 out]
                }
              }
            }
            n67 = call <resource>:"BaseProvider_IniFileSettings.vi"() -> ("IniFileSettings"=w77:T34)  [unwired: 18 in, 1 out]
            n68 = property class="VI"("Front Panel.Title"=w116) -> ()  [unwired: 2 in, 2 out]
            n69 = Unbundle By Name(w77) -> ("DynamicDispatchStartValue"=w76:bool, "UseGetSetForPropertyNodeMethods"=w72:bool)
            n70 = Select(t=u8 2 ("Disabled"), s=w87, f=u8 0 ("Disabled")) -> (s? t:f=w122:u8)
            n71 = Select(t=u8 2 ("Disabled"), s=w83, f=u8 0 ("Disabled")) -> (s? t:f=w82:u8)
            n72 = call <resource>:"AF_GetClassAfInfo.vi"("DeriveFromClassRef"=w97) -> ("AF Library Version"=w96:T36, "ClassType"=w94:T37)  [unwired: 5 in, 4 out]
            n73 = property on="Override Method" class="Bool (strict)"("Disabled"=w122) -> ()  [unwired: 2 in, 2 out]
            n74 = property on="Property Method" class="Bool (strict)"("DisabledEnum"=w82) -> ()  [unwired: 2 in, 2 out]
            n75 = case shown="\"Actor\"" w94 {
              tunnel: w96 -> [_ w178]
              tunnel: [_ w177] -> w95
              tunnel: [_ TRUE ("LimitToSpecificProviderTypeOfSameType(True)")] -> w93
              frame "NA", Default {
              }
              frame "Actor" {
                n76 = Unbundle(w178) -> ("Major"=w182:u16, "Minor"=w181:u16, "Fix"=w180:u16, "Build"=w179:u16)
                n77 = Format Into String(format string="%d.%d.%d.%d", w182, w181, w180, w179) -> (resulting string=w177:string)  [unwired: 2 in, 1 out]
              }
            }
            n78 = Select(t=enum16{"Read/Write Naming", "Get/Set Naming"}."Get/Set Naming" ("PropertyNodeMethodNaming"), s=w72, f=enum16{"Read/Write Naming", "Get/Set Naming"}."Read/Write Naming" ("PropertyNodeMethodNaming")) -> (s? t:f=w71:enum16{"Read/Write Naming", "Get/Set Naming"})
            n79 = local write "_DynamicDispatch"(w76) -> ()
            n80 = local write "PropertyNodeMethodNaming"(w71) -> ()
            n81 = property on="Property Node" class="Bool (strict)"("DisabledEnum"=w82) -> ()  [unwired: 2 in, 2 out]
            n82 = property on="PropertyNodeMethodNaming" class="Enum (strict)"("Visible"=FALSE) -> ()  [unwired: 2 in, 2 out]
            n83 = local write "_Visibility"(T7."Public" ("_Visibility")) -> ()
            n84 = property on=".vim" class="Bool (strict)"("Visible"=FALSE) -> ()  [unwired: 2 in, 2 out]
            n85 = Build Array (concatenate)(T22."invalid scope" ("Source Scope:Get"), w142) -> (w141:T33)
            n86 = Build Array (concatenate)("<class root>" ("Name"), w140) -> (w145:string[])
            n87 = Build Array (concatenate)(w110, w144) -> (w143:path[])
            n88 = property on="_Loading" class="Str"("Visible"=w125) -> ()  [unwired: 2 in, 2 out]
            n89 = property on="_AddMessageClass" class="Bool (strict)"("Visible"=w93, "DisabledEnum"=T19."Enabled" ("Disabled"), "Value"=TRUE ("LimitToSpecificProviderTypeOfSameType(True)")) -> ()  [unwired: 2 in, 2 out]
            n90 = property on="_MethodLocation" class="MCListbox (strict)"("TopLeft"=cluster{"Row":u32, "Column":u32} {"Row"=0, "Column"=0} ("Top Left Visible Cell")) -> ()  [unwired: 2 in, 2 out]
            n91 = Unbundle(T23 {"Left"=329, "Top"=250, "Right"=1119, "Bottom"=765} ("Front Panel Window:Panel Bounds")) -> ("Left"=w136:i16, "Top"=w134:i16, "Right"=w137:i16, "Bottom"=w135:i16)
            n92 = property class="VI"() -> ("Front Panel.PanelBounds"=w131:T23)  [unwired: 2 in, 2 out]
            n93 = Bundle By Name(cluster=w149, "FolderType"=w141, "FolderNames"=w145, "FolderPath"=w143, "ClassName"=w67, "AF"=w93, "ActorVersion"=w95, "MethodCaptionName"=w90, "Interface"=w83) -> (w151:T18)
            n94 = property on="_DubMethodName" class="Str"("Visible"=w125) -> ()  [unwired: 2 in, 2 out]
            n95 = Unbundle(w131) -> ("Left"=w130:i16, "Top"=w129:i16)  [unwired: 2 out]
            n96 = Subtract(x=w135, y=w134) -> (x-y=w132:i16)
            n97 = Subtract(x=w137, y=w136) -> (x-y=w133:i16)
            n98 = property on="_CreateMethod" class="Bool"("Disabled"=w117) -> ()  [unwired: 2 in, 2 out]
            n99 = Add(x=w130, y=w133) -> (x+y=w128:i16)
            n100 = Add(x=w129, y=w132) -> (x+y=w127:i16)
            n101 = local write "_MethodDescription"("" ("Method description")) -> ()
            n102 = Bundle(cluster=w131, "Left"=w130, "Top"=w129, "Right"=w128, "Bottom"=w127) -> (w126:T23)
            n103 = local write "_IconSize"(T20."Full" ("_IconSize")) -> ()
            n104 = property on="_CreateOpenClass" class="Bool"("Disabled"=w117) -> ()  [unwired: 2 in, 2 out]
            n105 = property on="MethodTemplateImage" class="Pict"("Visible"=w78) -> ()  [unwired: 2 in, 2 out]
            n106 = property class="VI"("Front Panel.PanelBounds"=w126) -> (error out=w86:errorcluster)  [unwired: 2 in, 1 out]
            n107 = property on="_Method" class="LstBox (strict)"("Selection Mode"=1) -> ()  [unwired: 2 in, 2 out]
            n108 = property on="_Method" class="LstBox (strict)"("Top Row"=u8 0 ("Disabled")) -> ()  [unwired: 2 in, 2 out]
            n109 = local write "_Method"(i32[] [0] ("_Method")) -> ()
            n110 = property on="ClearIcon" class="Bool"("Visible"=w78) -> ()  [unwired: 2 in, 2 out]
          }
          frame "GetTemplates" {
            n111 = call <resource>:"GetAllMethodsTypesForClass.vi"("ClassWriterNative"=w291, "ClassItemRefIn"=w288, "error in"=w290) -> ("DesignPattern"=w289:T10[], "NormalMethods"=w284:T12[], "OverrideMethods"=w287:T12[], "PropertyMethods"=w286:T12[], "ConnectorPaneHeight"=w283:i32[], "TemplateSettings"=w280:T17, "PropertyNodeMethods"=w282:T12[], "error out"=w264:errorcluster)  [unwired: 4 in, 1 out]
            n112 = Unbundle By Name(w280) -> ("OnlyNormalMethod"=w279:bool, "DynamicDispatch"=w275:enum8{"False", "True", "Mixed"}, "MustOverride"=w268:enum8{"False", "True", "Mixed"}, "MustCallParent"=w267:enum8{"False", "True", "Mixed"}, "OnlyPublic"=w266:bool)
            n113 = case shown="False" w266 {
              tunnel: [w297 w298] -> w265
              tunnel: [T19."Enabled" ("Disabled") w298] -> w262
              frame False {
                n114 = property on="_MethodLocation" class="MCListbox (strict)"() -> ("DisabledEnum"=w297:T19)  [unwired: 2 in, 2 out]
              }
              frame True {
                w298 = T19."Disabled and Grayed Out" ("Disabled")
              }
            }
            n115 = Array Size(array=w282) -> (size(s)=w281:i32)
            n116 = case shown="False" w279 {
              tunnel: w281 -> [w320 _]
              tunnel: [w319 T19."Enabled" ("Disabled")] -> w278
              tunnel: [T19."Enabled" ("Disabled") T19."Disabled and Grayed Out" ("Disabled")] -> w277
              tunnel: [T2."Normal Method" ("_MethodType") T2."Normal Method" ("_MethodType")] -> w276
              frame False {
                n117 = case shown="0" w320 {
                  tunnel: [T19."Enabled" ("Disabled") T19."Disabled and Grayed Out" ("Disabled")] -> w319
                  frame Default {
                  }
                  frame 0 {
                  }
                }
              }
              frame True {
              }
            }
            n118 = property on="_MethodLocation" class="MCListbox (strict)"("DisabledEnum"=w265) -> ()  [unwired: 2 in, 2 out]
            n119 = property on="_Visibility" class="RadioBtnsControl (strict)"("Disabled"=w262, "Value"=T7."Public" ("_Visibility")) -> ()  [unwired: 2 in, 2 out]
            n120 = for {
              tunnel: w284 -> [w329] mode=indexing
              tunnel: [w330] -> w285 mode=indexing
              tunnel: [w328] -> w260 mode=indexing
              tunnel: [w327] -> w261 mode=indexing
              tunnel: [w326] -> w257 mode=indexing
              n121 = Unbundle(w329) -> ("Name"=w328:string, "Path"=w327:path, "DynamicDispatch"=w326:T14)  [unwired: 3 out]
              n122 = case shown="\"\"" w328 {
                tunnel: [0 -1] -> w330
                frame Default {
                }
                frame "" {
                }
              }
            }
            n123 = case shown="\"Mixed\"" w275 {
              tunnel: [T19."Enabled" ("Disabled") T19."Disabled and Grayed Out" ("Disabled") T19."Disabled and Grayed Out" ("Disabled")] -> w274
              tunnel: [TRUE TRUE FALSE] -> w273
              frame "Mixed" {
              }
              frame "True" {
              }
              frame "False" {
              }
            }
            n124 = case shown="\"Mixed\"" w268 {
              tunnel: [T19."Enabled" ("Disabled") T19."Disabled and Grayed Out" ("Disabled") T19."Disabled and Grayed Out" ("Disabled")] -> w271
              tunnel: [FALSE TRUE FALSE] -> w272
              frame "Mixed" {
              }
              frame "True" {
              }
              frame "False" {
              }
            }
            n125 = case shown="\"Mixed\"" w267 {
              tunnel: [T19."Enabled" ("Disabled") T19."Disabled and Grayed Out" ("Disabled") T19."Disabled and Grayed Out" ("Disabled")] -> w270
              tunnel: [FALSE TRUE FALSE] -> w269
              frame "Mixed" {
              }
              frame "True" {
              }
              frame "False" {
              }
            }
            n126 = property on="_Method" class="LstBox (strict)"("Item Names"=w260, "Item Symbols"=w285) -> ()  [unwired: 2 in, 2 out]
            n127 = Bundle By Name(cluster=w259, "DesignPatterns"=w289, "NormalMethods"=w284, "OverrideMethods"=w287, "PropertyMethods"=w286, "MethodVIs"=w261, "MethodItemNames"=w260, "ConnectorPaneHeight"=w283, "PropertyNodeMethods"=w282, "TemplateSettings"=w280, "Methods.DynamicDispatch"=w257) -> (w293:T18)
            n128 = Array Size(array=w284) -> (size(s)=w292:i32)
            n129 = property on="_MethodType" class="RadioBtnsControl (strict)"("DisabledEnum"=w277, "Value"=w276) -> ()  [unwired: 2 in, 2 out]
            n130 = property on="_DynamicDispatch" class="Bool (strict)"("Disabled"=w274, "Value"=w273) -> ()  [unwired: 2 in, 2 out]
            n131 = property on="_MustOverride" class="Bool (strict)"("Disabled"=w271, "Value"=w272) -> ()  [unwired: 2 in, 2 out]
            n132 = property on="_MustCallParent" class="Bool (strict)"("Disabled"=w270, "Value"=w269) -> ()  [unwired: 2 in, 2 out]
            n133 = Unbundle By Name(w259) -> ("Interface"=w258:bool)
            n134 = case shown="1.." w292 {
              tunnel: ["Exit" "UpdateScopeList"] -> w294
              frame 0, Default {
                n135 = One Button Dialog(message="No method templates where found for this class" ("format string")) -> ()  [unwired: 1 in, 1 out]
              }
              frame 1.. {
              }
            }
            n136 = case shown="False" w258 {
              tunnel: w278 -> [w295 _]
              frame False {
                n137 = property on="Property Node" class="Bool (strict)"("DisabledEnum"=w295) -> ()  [unwired: 2 in, 2 out]
              }
              frame True {
              }
            }
          }
          frame "UpdateScopeList" {
            n138 = property class="LVClassLibrary"(reference=w350) -> ("Path"=w345:path)  [unwired: 1 in, 2 out]
            n139 = Unbundle By Name(w342) -> ("FolderNames"=w348:string[], "FolderPath"=w349:path[], "FolderType"=w347:T33)
            n140 = Strip Path(path=w345) -> (stripped path=w344:path)  [unwired: 1 out]
            n141 = for {
              tunnel: w349 -> [w365] mode=indexing
              tunnel: w344 -> [w364]
              tunnel: w348 -> [w351] mode=indexing
              tunnel: w347 -> [w355] mode=indexing
              tunnel: [w357] -> w339 mode=indexing
              tunnel: [w352] -> w340 mode=indexing
              n142 = Path To String(path=w364) -> (string=w362:string)
              n143 = Path To String(path=w365) -> (string=w363:string)
              n144 = Search and Replace String(input string=w363, search string=w362) -> (result string=w361:string)  [unwired: 6 in, 3 out]
              n145 = case shown="Default" w355 {
                selector: w355 -> [_ w368]
                tunnel: ["<any scope>" w367] -> w354
                frame "invalid scope" {
                }
                frame Default {
                  n146 = Format Into String(w368) -> (resulting string=w367:string)  [unwired: 3 in, 1 out]
                }
              }
              n147 = String Subset(string=w361, offset (0)=1) -> (substring=w353:string)  [unwired: 1 in]
              n148 = String To Path(string=w353) -> (path=w352:path)
              n149 = Empty String/Path?(string/path=w353) -> (empty?=w359:bool)
              n150 = Select(t=".", s=w359, f=w353) -> (s? t:f=w356:string)
              n151 = Build Array(w351, w356, w354) -> (w357:string[])
            }
            n152 = Bundle By Name(cluster=w342, "RelFolderPath"=w340, "MethodLocation"=w339) -> (w341:T18)
            n153 = property on="_MethodLocation" class="MCListbox (strict)"("ItemNames"=w339, "Value"=0 ("Method Location")) -> ()  [unwired: 2 in, 2 out]
            n154 = call <resource>:"GDSString_AddStatesToQueue.vi"("EmptyQueueNextState"="GetCurrentClassMethods", "State(s) in (\"\")"=w336) -> ("States Out"=w337:string)  [unwired: 13 in]
          }
          frame "GetCurrentClassMethods" {
            n155 = invoke class="LVClassLibrary" method="Get All Descendents"(reference=w372, error in=w370, "Type"="VI") -> (error out=w369:errorcluster, "All Descendents"=w373:refnum<vi>[])  [unwired: 4 in, 5 out]
            n156 = for {
              tunnel: w373 -> [w387] mode=indexing
              tunnel: [w379] -> w371 mode=indexing
              n157 = property class="ProjectItem"(reference=w387) -> (reference out=w382:refnum<vi>, error out=w384:errorcluster, "Reference"=w381:refnum<vi>)  [unwired: 1 in]
              n158 = property class="VI"(reference=w381, error in=w384) -> (reference out=w385:refnum<vi>, error out=w386:errorcluster, "Name"=w380:string)
              n159 = Close Reference(reference=w385, error in (no error)=w386) -> (error out=w383:errorcluster)
              n160 = Close Reference(reference=w382, error in (no error)=w383) -> ()  [unwired: 1 out]
              n161 = Match Pattern(string=w380, regular expression=":") -> (after substring=w379:string)  [unwired: 1 in, 3 out]
            }
            n162 = Bundle By Name(cluster=w377, "ClassVIs"=w371) -> (w376:T18)
          }
          frame "GetClassColors" {
            w421 = u8 32 ("x")
            n163 = Unbundle By Name(w396) -> ("Interface"=w395:bool)
            n164 = call <resource>:"GDSLvClass_ReadClassColors.vi"("Library Refnum"=w400, "error in (no error)"=w431) -> ("LvClassIconSettings"=w412:T38, "error out"=w422:errorcluster)  [unwired: 12 in, 4 out]
            n165 = Unbundle By Name(w412) -> ("ColorProtected"=w409:u32, "ColorPrivate"=w410:u32, "ColorPublic"=w405:u32, "Frame"=w411:u32, "Frame thickness"=w408:u8, "Body Text"=w407:u32)
            n166 = case shown="True" w395 {
              tunnel: w422 -> [w432 w444]
              tunnel: w400 -> [w433 w443]
              tunnel: [w433 w442] -> w397
              tunnel: [_ w440] -> w394
              tunnel: [_ w439] -> w393
              tunnel: [_ w438] -> w392
              tunnel: [w432 w435] -> w391
              tunnel: [_ w434] -> w389
              frame True {
              }
              frame False {
                n167 = property class="LVClassLibrary"(reference=w443, error in=w444) -> (reference out=w442:refnum<vi>, error out=w441:errorcluster, "Member Data"=w437:refnum<vi>)
                n168 = call <resource>:"GDSLvIcon_AnalyseViIcon.vi"("ViRef/LvCLassRef/LvLibRef/ViPath/2D_Image"=w437, "error in (no error)"=w441) -> ("Splitter0px"=w434:bool, "ValidHeaderIcon"=w440:bool, "HeaderIcon"=w439:u8[][], "HeaderBkColor"=w438:u32, "error out"=w436:errorcluster)  [unwired: 4 in, 9 out]
                n169 = Close Reference(reference=w437, error in (no error)=w436) -> (error out=w435:errorcluster)
              }
            }
            n170 = Equal?(x=w405, y=w407) -> (x = y?=w418:bool)
            n171 = Bundle(FALSE, "ColorPublic"=w405) -> (w406:cluster{bool, "ColorPublic":u32})  [unwired: 1 in]
            n172 = Equal?(x=u32 0 ("Frame"), y=w405) -> (x = y?=w417:bool)
            n173 = local write "_BodyBk"(w406) -> ()
            n174 = Select(t=u32 16777215 ("Frame"), s=w417, f=u32 0 ("Frame")) -> (s? t:f=w413:u32)
            n175 = Select(t=w413, s=w418, f=w407) -> (s? t:f=w402:u32)
            n176 = Bundle(FALSE, "Body Text"=w402) -> (w401:cluster{bool, "Body Text":u32})  [unwired: 1 in]
            n177 = local write "_BodyText"(w401) -> ()
            n178 = case shown="False" w394 {
              tunnel: w393 -> [_ w463]
              tunnel: w392 -> [_ w462]
              tunnel: [w448 w463] -> w399
              tunnel: [w449 w462] -> w398
              tunnel: w391 -> [w455 w461]
              tunnel: w397 -> [w454 _]
              tunnel: [w453 w461] -> w390
              tunnel: w389 -> [_ w460]
              tunnel: [w445 w460] -> w388
              frame False {
                n179 = call <resource>:"GDSLvIcon_AnalyseViIcon.vi"("ViRef/LvCLassRef/LvLibRef/ViPath/2D_Image"=w454, "error in (no error)"=w455) -> ("Splitter0px"=w445:bool, "ValidHeaderIcon"=w452:bool, "HeaderIcon"=w451:u8[][], "HeaderBkColor"=w450:u32, "BodyIcon"=w447:u8[][], "BodyBkColor"=w446:u32, "error out"=w453:errorcluster)  [unwired: 4 in, 7 out]
                n180 = case shown="False" w452 {
                  tunnel: w451 -> [_ w458]
                  tunnel: [w456 w459] -> w449
                  tunnel: w450 -> [_ w459]
                  tunnel: [w457 w458] -> w448
                  tunnel: w447 -> [w457 _]
                  tunnel: w446 -> [w456 _]
                  frame False {
                  }
                  frame True {
                  }
                }
              }
              frame True {
              }
            }
            n181 = Array Size(array=w399) -> (size(s)=w428:i32[])
            n182 = Multiply(x=w408, y=u8 2) -> (x*y=w424:u8)
            n183 = Index Array(array=w428) -> (element #1=w425:i32)  [unwired: 2 in, 1 out]
            n184 = Add(x=w425, y=w424) -> (x+y=w423:i32)
            n185 = Increment(x=w423) -> (x+1=w420:i32)
            n186 = Subtract(x=w421, y=w420) -> (x-y=w419:i32)
            n187 = Subtract(x=w421, y=w424) -> (x-y=w426:u8)
            n188 = Bundle By Name(cluster=w396, "ColorProtected"=w409, "ColorPrivate"=w410, "ColorPublic"=w405, "Frame"=w411, "Frame thickness"=w408, "HeaderBkColor"=w398, "HeaderIcon"=w399, "BodyIconHeight"=w419, "BodyIconWidth"=w426, "Splitter0px"=w388) -> (w430:T18)
          }
          frame "UpdateMethodSignatures" {
            w479 = 0  # Current
            w481 = string[] []  # SignatureText
            w482 = string[] []  # SignatureName
            n189 = call <resource>:"GOOP_GetGDSConfigFolder.vi"() -> ("GDSFolderPath"=w486:path)
            n190 = Build Path(base path=w486, name or relative path="MethodSignatures.xml") -> (appended path=w484:path)
            n191 = Read from Text File(file (use dialog)=w484) -> (text=w483:string)  [unwired: 3 in, 3 out]
            n192 = Bundle("SignatureName"=w482, "SignatureText"=w481, "Current"=w479) -> (w480:T39)  [unwired: 1 in]
            n193 = Unflatten From XML(xml string=w483, type=w480) -> (value=w478:T39)  [unwired: 1 in, 1 out]
            n194 = Unbundle By Name(w469) -> ("Signatures.Current"=w465:i32)
            n195 = Unbundle By Name(w478) -> ("SignatureName"=w473:string[], "Current"=w471:i32, "SignatureText"=w464:string[])
            n196 = Greater Or Equal To 0?(x=w465) -> (x >= 0?=w468:bool)
            n197 = Array Size(array=w473) -> (size(s)=w472:i32)
            n198 = Bundle By Name(cluster=w469, "Signatures"=w478) -> (w467:T18)
            n199 = Max & Min(x=w472, y=w471) -> (min(x,y)=w470:i32)  [unwired: 1 out]
            n200 = case shown="False" w468 {
              tunnel: w467 -> [w488 w491]
              tunnel: [w488 w490] -> w466
              tunnel: w465 -> [_ w489]
              frame False {
              }
              frame True {
                n201 = Bundle By Name(cluster=w491, "Signatures.Current"=w489) -> (w490:T18)
              }
            }
            n202 = Build Array (concatenate)("No signature", w473, string[] ["-", "Add signature"] ("array")) -> (w474:string[])
            n203 = case shown="1.." w470 {
              selector: w470 -> [_ w496]
              tunnel: w464 -> [_ w495]
              frame 0, Default {
              }
              frame 1.. {
                n204 = Decrement(x=w496) -> (x-1=w492:i32)
                n205 = Index Array(array=w495, index=w492) -> (element=w494:string)
                n206 = call <resource>:"UpdateMethodSignatureText.vi"("TagCodedStringIn"=w494) -> ("StringOut"=w493:string)  [unwired: 10 in]
                n207 = local write "_MethodDescription"(w493) -> ()
              }
            }
            n208 = property on="_MethodSignature" class="Ring (strict)"("Strings []"=w474, "Value"=w470) -> ()  [unwired: 2 in, 2 out]
          }
          frame "", "Idle" {
            (unwired) "UpdateMethodSettings"
            (unwired) "Idle"
            (unwired) ""
            n209 = event shown="[3] \"_MethodIcons\": Value Change" {
              selector: _ -> [_ _ _ _ _ _ _ _ _ _ _ _ _ _ _ _ _ _ _ _ _ _ _ _ _ _ _ _ _ _ _ _ _ _ _]
              dyn-events: _ -> [_ _ _ _ _ _ _ _ _ _ _ _ _ _ _ _ _ _ _ _ _ _ _ _ _ _ _ _ _ _ _ _ _ _ _]
              timeout: _ -> [_ _ _ _ _ _ _ _ _ _ _ _ _ _ _ _ _ _ _ _ _ _ _ _ _ _ _ _ _ _ _ _ _ _ _]
              tunnel: [w564 w614 w637 w714 "Generate icon" w732 "Idle" w797 "Exit" "Exit" w851 w879 "UpdateIconFromParentMethod" "Idle" w974 "Idle" "UpdateMethodSettings\nUpdateIcon" _ "UpdateIcon" w1284 "Idle" "Idle" w1357 "Idle" "UpdateIcon" "UpdateMethodSettings\nUpdateIcon" "UpdateIcon" w1460 "UpdateMethodSettings\nUpdateIcon" "Idle" w1560 _ "UpdateMethodSettings" ("y") "Idle" "Idle"] -> w515
              tunnel: [_ _ _ _ _ _ _ _ TRUE w841 _ _ _ _ _ _ _ _ _ _ _ _ _ _ _ _ _ _ _ _ _ _ _ _ _] -> w513
              tunnel: w502 -> [w569 _ w639 w709 _ w734 w779 w795 _ _ _ _ w939 w958 _ _ w1039 _ _ w1286 w1342 w1349 w1356 w1381 _ w1397 _ w1459 w1463 w1502 w1540 w1631 _ _ _]
              tunnel: [_ _ _ _ _ _ _ _ _ _ "_CreateOpenClass" _ _ _ _ _ _ _ _ _ _ _ _ _ _ _ _ _ _ _ _ _ _ _ _] -> w512
              tunnel: w502 -> [w573 w620 w641 w712 w726 w736 w783 w785 w836 w840 w852 w870 w932 w961 w980 w1009 w1020 w1279 w1281 w1289 w1346 w1352 w1359 w1384 w1395 w1404 w1452 w1461 w1470 w1503 w1543 w1633 w1647 w1649 w1653]
              tunnel: [w572 w620 w640 w713 w727 w735 w782 w785 w836 w840 w852 w869 w932 w957 w979 w1009 w1019 w1279 w1281 w1288 w1345 w1351 w1358 w1383 w1393 w1404 w1452 w1461 w1470 w1503 w1542 w1632 w1647 w1649 w1653] -> w511
              tunnel: [_ _ _ _ _ w731 w778 _ _ _ _ _ w930 _ _ _ _ _ _ _ _ w1348 w1355 w1380 _ _ _ w1455 _ w1501 _ _ _ _ _] -> w501
              tunnel: [w570 w619 w621 w711 w729 w730 w777 w784 w835 w839 w843 w863 w931 w960 w977 w1008 w1016 w1278 w1280 w1283 w1340 w1347 w1354 w1379 w1391 w1396 w1451 w1454 w1462 w1500 w1524 w1640 w1646 w1648 w1652] -> w500
              tunnel: w499 -> [w570 w619 w621 w710 w729 w730 w777 w784 w835 w839 w843 w863 w931 w960 w976 w1008 w1016 w1278 w1280 w1283 w1340 w1347 w1354 w1379 w1391 w1396 w1451 w1454 w1462 w1500 w1524 w1640 w1646 w1648 w1652]
              tunnel: w498 -> [_ w613 _ _ _ _ _ _ _ _ _ _ _ _ _ _ _ _ _ _ _ _ _ _ _ _ _ _ _ _ _ _ _ _ _]
              tunnel: [_ w613 _ _ _ _ _ _ _ _ _ _ _ _ _ _ _ _ _ _ _ _ _ _ _ _ _ _ _ _ _ _ _ _ _] -> _
              tunnel: w497 -> [_ _ _ _ _ _ _ _ _ _ _ _ _ _ w975 _ _ _ _ _ _ _ _ _ _ _ _ _ _ _ _ _ _ _ _]
              tunnel: [_ _ _ _ _ _ _ _ _ _ _ _ _ _ _ _ _ _ _ _ _ _ _ _ _ _ _ _ _ _ _ w1628 _ _ _] -> _
              event "_Method": Value Change {
                n210 = event-data() -> ()  [unwired: 1 in, 1 out]
                n211 = local read "_MethodType"() -> (w574:T2)
                n212 = case shown="\"Property Method\", \"Property Node\"" w574 {
                  selector: w574 -> [_ _ w597]
                  tunnel: "_Method" -> [_ _ w601]
                  tunnel: ["UpdateMethodTemplateImage" "UpdateMethodTemplateImage" "UpdateMethodTemplateImage\nUpdateIcon"] -> w565
                  tunnel: w569 -> [_ _ _]
                  tunnel: [_ _ w598] -> w571
                  tunnel: [_ _ w589] -> w560
                  frame "Normal Method" {
                  }
                  frame "Override Method" {
                  }
                  frame "Property Method", "Property Node" {
                    n213 = call <resource>:"BaseProvider_IniFileSettings.vi"() -> ("IniFileSettings"=w592:T34)  [unwired: 18 in, 1 out]
                    n214 = local read "_Property"() -> (w590:string[])
                    n215 = local read "PropertyNodeMethodNaming"() -> (w586:enum16{"Read/Write Naming", "Get/Set Naming"})
                    n216 = Unbundle By Name(w592) -> ("FileNamingOption"=w591:T35)
                    n217 = Equal?(x=w597, y=T2."Property Node") -> (x = y?=w588:bool)
                    n218 = for {
                      tunnel: w590 -> [w605] mode=indexing
                      tunnel: [w602] -> w589
                      stop <- w602 stop-if-true
                      n219 = Match Pattern(string=w605, regular expression="^ClassAttribute" ("Left Cell String(Main name)")) -> (offset past match=w603:i32)  [unwired: 1 in, 3 out]
                      n220 = Greater Or Equal To 0?(x=w603) -> (x >= 0?=w602:bool)
                    }
                    n221 = property on="_Method" class="LstBox (strict)"() -> ("Item Names"=w599:string[])  [unwired: 2 in, 2 out]
                    n222 = Equal?(x=w586, y=enum16{"Read/Write Naming", "Get/Set Naming"}."Read/Write Naming") -> (x = y?=w584:bool)
                    n223 = Compound Arithmetic op=AND(w584, w588) -> (w587:bool)
                    n224 = call <resource>:"CreateMethodNames.vi"("_Method"=w601, "FileNamingOption"=w591, "_Property"=w590, "Item Names"=w599, "Use Read/Write"=w587) -> ("MethodNames"=w598:string[], "Attribute/PropertyNames"=w594:string[])
                    n225 = Index Array(array=w598) -> (element=w595:string)  [unwired: 1 in]
                    n226 = case shown="True" w588 {
                      tunnel: w595 -> [w606 _]
                      tunnel: [w606 w607] -> w593
                      tunnel: w594 -> [_ w611]
                      frame False {
                      }
                      frame True {
                        n227 = Array To Spreadsheet String(delimiter (Tab)="/", array=w611, 3:"%s" ("format string")) -> (spreadsheet string=w608:string)
                        n228 = call <vilib>:"Trim Whitespace.vi"("string"=w608) -> ("trimmed string"=w607:string)  [unwired: 1 in]
                      }
                    }
                    n229 = local write "_MethodIconName"(w595) -> ()
                    n230 = local write "_MethodName"(w593) -> ()
                  }
                }
                n231 = Unbundle By Name(w569) -> ("Methods.DynamicDispatch"=w567:T14[])
                n232 = Index Array(array="_Method") -> (element=w566:i32)  [unwired: 1 in]
                n233 = Index Array(array=w567, index=w566) -> (element=w559:T14)
                n234 = case shown="\"Default\", Default" w559 {
                  tunnel: w560 -> [w575 _ _ _ _]
                  frame "Default", Default {
                    n235 = case shown="False" w575 {
                      frame False {
                        n236 = call <resource>:"BaseProvider_IniFileSettings.vi"() -> ("IniFileSettings"=w577:T34)  [unwired: 18 in, 1 out]
                        n237 = Unbundle By Name(w577) -> ("DynamicDispatchStartValue"=w576:bool)
                        n238 = local write "_DynamicDispatch"(w576) -> ()
                      }
                      frame True {
                      }
                    }
                  }
                  frame "OnAtStart" {
                    n239 = local write "_DynamicDispatch"(TRUE ("_DynamicDispatch")) -> ()
                  }
                  frame "OffAtStart" {
                    n240 = local write "_DynamicDispatch"(FALSE ("_DynamicDispatch")) -> ()
                  }
                  frame "AlwaysOn" {
                    n241 = local write "_DynamicDispatch"(TRUE ("_DynamicDispatch")) -> ()
                  }
                  frame "AlwaysOff" {
                    n242 = local write "_DynamicDispatch"(FALSE ("_DynamicDispatch")) -> ()
                  }
                }
                n243 = call "Is Value Changed.vim"("value"=w559) -> ("changed or first call?"=w558:bool)
                n244 = Select(t="UpdateMethodSettings", s=w558, f="") -> (s? t:f=w561:string)
                n245 = Bundle By Name(cluster=w573, "MethodNames"=w571) -> (w572:T18)
                n246 = call <resource>:"GDSString_AddStatesToQueue.vi"("State(s) in (\"\")"=w565, "State(s) at Back (\"\")"=w561) -> ("States Out"=w564:string)  [unwired: 13 in]
              }
              event "_Method": Mouse Enter; "_Method": Mouse Leave {
                n247 = event-data() -> ("Type"=w618:T24)  [unwired: 1 in]
                n248 = Equal?(x=lveventtype."Mouse Enter" ("y"), y=w618) -> (x = y?=w617:bool)
                n249 = property on="MethodTemplateImage" class="Pict"("Visible"=w617) -> ()  [unwired: 2 in, 2 out]
                n250 = Select(t="UpdateMethodTemplateImage", s=w617, f="Idle") -> (s? t:f=w614:string)
              }
              event Key Down? {
                (unwired) TRUE
                n251 = event-data() -> ("VKey"=w636:T40, "PlatMods.Ctrl"=w625:bool)  [unwired: 1 in]
                n252 = property on="_MethodName" class="Str"() -> ("Key Focus"=w622:bool)  [unwired: 2 in, 2 out]
                n253 = property on="_FontCompression" class="Enum (strict)"() -> ("Key Focus"=w635:bool)  [unwired: 2 in, 2 out]
                n254 = property on="_TextAlignment" class="Ring (strict)"() -> ("Key Focus"=w634:bool)  [unwired: 2 in, 2 out]
                n255 = property on="_IconSize" class="Ring (strict)"() -> ("Key Focus"=w633:bool)  [unwired: 2 in, 2 out]
                n256 = property on="_MethodLocation" class="MCListbox (strict)"() -> ("Key Focus"=w632:bool)  [unwired: 2 in, 2 out]
                n257 = property on="_OverrideMethods" class="LstBox (strict)"() -> ("Key Focus"=w631:bool)  [unwired: 2 in, 2 out]
                n258 = property on="_Property" class="Tree (strict)"() -> ("Key Focus"=w630:bool)  [unwired: 2 in, 2 out]
                n259 = property on="_MethodDescription" class="Str"() -> ("Key Focus"=w629:bool)  [unwired: 2 in, 2 out]
                n260 = property on="_MethodIconName" class="Str"() -> ("Key Focus"=w628:bool)  [unwired: 2 in, 2 out]
                n261 = property on="_Method" class="LstBox (strict)"() -> ("Key Focus"=w627:bool)  [unwired: 2 in, 2 out]
                n262 = property on="_MethodSignature" class="Ring (strict)"() -> ("Key Focus"=w626:bool)  [unwired: 2 in, 2 out]
                n263 = Unbundle By Name(w639) -> ("Offset.X"=w643:i32, "Offset.Y"=w642:i32)
                n264 = Compound Arithmetic op=OR(w635, w634, w633, w632, w631, w630, w630, w629, w628, w627, w626, w622) -> (w624:bool)
                n265 = Compound Arithmetic op=OR(w625, invert w624) -> (w623:bool)
                n266 = case shown="True" w623 {
                  tunnel: w641 -> [w645 w649]
                  tunnel: [w645 w653] -> w640
                  tunnel: w636 -> [_ w652]
                  tunnel: w642 -> [_ w646]
                  tunnel: w643 -> [_ w647]
                  tunnel: ["Idle" w651] -> w637
                  tunnel: [_ w650] -> w638
                  frame False {
                  }
                  frame True {
                    n267 = Bundle By Name(cluster=w649, "OldOffset.X"=w647, "OldOffset.Y"=w646) -> (w648:T18)
                    n268 = case shown="\"Right\"" w652 {
                      tunnel: w648 -> [w660 w662 w669 w676 w683]
                      tunnel: [w659 w662 w668 w675 w682] -> w653
                      tunnel: w646 -> [w658 _ w667 w673 w680]
                      tunnel: w647 -> [w656 _ w665 w674 w681]
                      tunnel: ["UpdateIcon" "Idle" "UpdateIcon" "UpdateIcon" "UpdateIcon"] -> w651
                      tunnel: [TRUE _ TRUE TRUE TRUE] -> w650
                      frame "Up" {
                        n269 = Decrement(x=w658) -> (x-1=w657:i32)
                        n270 = Bundle By Name(cluster=w660, "Offset.X"=w656, "Offset.Y"=w657) -> (w659:T18)
                      }
                      frame Default {
                      }
                      frame "Down" {
                        n271 = Increment(x=w667) -> (x+1=w666:i32)
                        n272 = Bundle By Name(cluster=w669, "Offset.X"=w665, "Offset.Y"=w666) -> (w668:T18)
                      }
                      frame "Left" {
                        n273 = Decrement(x=w674) -> (x-1=w672:i32)
                        n274 = Bundle By Name(cluster=w676, "Offset.X"=w672, "Offset.Y"=w673) -> (w675:T18)
                      }
                      frame "Right" {
                        n275 = Increment(x=w681) -> (x+1=w679:i32)
                        n276 = Bundle By Name(cluster=w683, "Offset.X"=w679, "Offset.Y"=w680) -> (w682:T18)
                      }
                    }
                  }
                }
                n277 = event-data("Discard?"=w638) -> ()  [unwired: 1 in, 1 out]
              }
              event "_MethodIcons": Value Change {
                n278 = event-data() -> ()  [unwired: 1 in, 1 out]
                n279 = Unbundle By Name(w709) -> ("HeaderIcon"=w685:u8[][])
                n280 = Unbundle By Name(w709) -> ("RowStart(0)"=w695:i32, "ImageRows(32)"=w696:i32, "Frame thickness"=w694:i32, "Frame"=w697:u32)
                n281 = Unbundle By Name(w709) -> ("BodyIconHeight"=w700:i32, "BodyIconWidth"=w701:i32, "HeaderBkColor"=w702:u32, "Offset"=w708:cluster{"X":i32, "Y":i32}, "CurrentIcon"=w684:T29)
                n282 = local read "_FontCompression"() -> (w689:enum16{"Auto", "On", "Off"})
                n283 = local read "_MethodIconName"() -> (w691:string)
                n284 = local read "_TextAlignment"() -> (w688:u16)
                n285 = local read "_CapitalOnly"() -> (w690:bool)
                n286 = local read "_BodyText"() -> (w687:T1)
                n287 = local read "_BodyBk"() -> (w686:T1)
                n288 = Unbundle By Name(w687) -> ("Color"=w698:u32)
                n289 = Unbundle By Name(w686) -> ("Color"=w699:u32)
                n290 = Bundle By Name(cluster=T25 {"HeaderIcon"=[], "RowStart(0)"=0, "ImageRows(32)"=32, "FrameThickness(1)"=1, "FrameColor"=0, "IconTextDataType"={"Text"="", "Allow Only Capital Chars"=FALSE, "Compression"=enum."Auto", "Alignment"=enum."Center"}, "BodyTextColor"=0, "BodyBackgroundColor"=0, "BodyIconHeight"=0, "BodyIconWidth"=0, "HeaderBackgroundColor"=0, "BodyIcon"=[[0, 0, 0, 0, 0, 0, 0, 0, 0, 0, 255, 255, 0, 0, 255, 0, 0, 0, 255, 0, 0, 0, 0, 0, 0, 0, 0, 0, 0, 0], [0, 0, 0, 0, 0, 0, 0, 0, 0, 255, 0, 0, 255, 0, 255, 0, 0, 0, 255, 0, 0, 0, 0, 0, 0, 0, 0, 0, 0, 0], [0, 0, 0, 0, 0, 0, 0, 0, 0, 255, 255, 255, 255, 0, 255, 0, 0, 0, 255, 0, 0, 0, 0, 0, 0, 0, 0, 0, 0, 0], [0, 0, 0, 0, 0, 0, 0, 0, 0, 255, 0, 0, 255, 0, 255, 0, 0, 0, 255, 0, 0, 0, 0, 0, 0, 0, 0, 0, 0, 0], [0, 0, 0, 0, 0, 0, 0, 0, 0, 255, 0, 0, 255, 0, 255, 255, 255, 0, 255, 255, 255, 0, 0, 0, 0, 0, 0, 0, 0, 0], [0, 0, 255, 0, 0, 0, 255, 0, 0, 255, 255, 0, 0, 255, 0, 0, 255, 0, 255, 255, 0, 255, 255, 0, 0, 0, 255, 255, 0, 0], [0, 255, 0, 255, 0, 255, 0, 255, 0, 255, 0, 255, 0, 255, 255, 0, 255, 0, 255, 0, 0, 255, 0, 255, 0, 255, 0, 0, 0, 0], [0, 255, 0, 0, 0, 255, 0, 255, 0, 255, 255, 0, 0, 255, 0, 255, 255, 0, 255, 255, 0, 255, 255, 0, 0, 0, 255, 0, 0, 0], [0, 255, 0, 255, 0, 255, 0, 255, 0, 255, 0, 255, 0, 255, 0, 0, 255, 0, 255, 0, 0, 255, 0, 255, 0, 0, 0, 255, 0, 0], [0, 0, 255, 0, 0, 0, 255, 0, 0, 255, 0, 255, 0, 255, 0, 0, 255, 0, 255, 255, 0, 255, 0, 255, 0, 255, 255, 0, 0, 0], [0, 255, 0, 0, 0, 255, 0, 0, 255, 0, 0, 255, 0, 255, 0, 0, 255, 0, 255, 255, 0, 0, 255, 0, 0, 255, 255, 255, 0, 255], [255, 0, 255, 0, 255, 0, 255, 0, 255, 255, 0, 255, 0, 255, 255, 0, 255, 0, 255, 0, 0, 255, 0, 255, 0, 0, 255, 0, 0, 255], [255, 0, 0, 0, 255, 0, 255, 0, 255, 0, 255, 255, 0, 255, 0, 255, 255, 0, 255, 255, 0, 255, 0, 0, 0, 0, 255, 0, 0, 255], [255, 0, 255, 0, 255, 0, 255, 0, 255, 0, 0, 255, 0, 255, 0, 0, 255, 0, 255, 0, 0, 255, 0, 255, 0, 0, 255, 0, 0, 255], [0, 255, 0, 0, 0, 255, 0, 0, 255, 0, 0, 255, 0, 255, 0, 0, 255, 0, 255, 255, 0, 0, 255, 0, 0, 0, 255, 0, 0, 255], [0, 0, 0, 0, 0, 0, 0, 0, 0, 0, 0, 0, 0, 0, 255, 0, 0, 0, 0, 0, 0, 0, 0, 0, 0, 0, 0, 0, 0, 0], [0, 0, 0, 0, 0, 0, 0, 0, 0, 0, 0, 0, 0, 255, 0, 0, 0, 0, 0, 0, 0, 0, 0, 0, 0, 0, 0, 0, 0, 0], [0, 0, 0, 0, 0, 0, 0, 0, 0, 0, 0, 0, 0, 255, 255, 0, 0, 0, 0, 0, 0, 0, 0, 0, 0, 0, 0, 0, 0, 0], [0, 0, 0, 0, 0, 0, 0, 0, 0, 0, 0, 0, 0, 255, 0, 255, 0, 0, 0, 0, 0, 0, 0, 0, 0, 0, 0, 0, 0, 0], [0, 0, 0, 0, 0, 0, 0, 0, 0, 0, 0, 0, 0, 0, 255, 0, 0, 0, 0, 0, 0, 0, 0, 0, 0, 0, 0, 0, 0, 0], [0, 0, 0, 0, 0, 0, 0, 0, 0, 0, 0, 0, 0, 0, 0, 0, 0, 0, 0, 0, 0, 0, 0, 0, 0, 0, 0, 0, 0, 0], [0, 0, 0, 0, 0, 0, 0, 0, 0, 0, 0, 0, 0, 0, 0, 0, 0, 0, 0, 0, 0, 0, 0, 0, 0, 0, 0, 0, 0, 0]], "Offset"={"X"=0, "Y"=0}, "CurrentIcon"={"BgIcon"=[], "BgIconOffset"={"X"=0, "Y"=0}, "BgIconMask"=[], "ColorsOkayforiconToBeOnTopOf"=[]}} ("IconInfo"), "HeaderIcon"=w685, "RowStart(0)"=w695, "ImageRows(32)"=w696, "FrameThickness(1)"=w694, "FrameColor"=w697, "IconTextDataType.Text"=w691, "IconTextDataType.Allow Only Capital Chars"=w690, "IconTextDataType.Compression"=w689, "IconTextDataType.Alignment"=w688, "BodyTextColor"=w698, "BodyBackgroundColor"=w699, "BodyIconHeight"=w700, "BodyIconWidth"=w701, "HeaderBackgroundColor"=w702, "Offset"=w708, "CurrentIcon"=w684) -> (w693:T25)
                n291 = call <resource>:"GDSIconEditor_IconDialog.vi"("error in (no error)"=w710, "IconInfo"=w693) -> ("error out"=w711:errorcluster, "Icon exist"=w707:bool, "CurrentIcon"=w706:T29, "Cancelled"=w705:bool, "Offset"=w704:cluster{"X":i32, "Y":i32}, "BodyIcon"=w703:u8[][])  [unwired: 4 in]
                n292 = case shown="False" w705 {
                  tunnel: w712 -> [w721 w722]
                  tunnel: [w720 w722] -> w713
                  tunnel: w703 -> [w719 _]
                  tunnel: w704 -> [w718 _]
                  tunnel: w706 -> [w717 _]
                  tunnel: w707 -> [_ _]
                  tunnel: ["Generate icon" _] -> w714
                  frame False {
                    n293 = Bundle By Name(cluster=w721, "BodyIcon"=w719, "Offset"=w718, "CurrentIcon"=w717) -> (w720:T18)
                    n294 = property on="ClearIcon" class="Bool"("Visible"=TRUE) -> ()  [unwired: 2 in, 2 out]
                  }
                  frame True {
                  }
                }
              }
              event "ClearIcon": Value Change {
                n295 = event-data() -> ()  [unwired: 1 in, 6 out]
                n296 = property on="ClearIcon" class="Bool"("Visible"=FALSE) -> ()  [unwired: 2 in, 2 out]
                n297 = Bundle By Name(cluster=w726, "BodyIcon"=u8[][] [], "CurrentIcon"=T29 {"BgIcon"=[], "BgIconOffset"={"X"=0, "Y"=0}, "BgIconMask"=[], "ColorsOkayforiconToBeOnTopOf"=[]}) -> (w727:T18)
              }
              event Mouse Move {
                n298 = event-data() -> ("Coords"=w733:T15)  [unwired: 1 in]
                n299 = Unbundle By Name(w734) -> ("DraggingText"=w738:bool, "DraggingIcon"=w737:bool)
                n300 = Unbundle By Name(w734) -> ("OverrideMethod"=w731:path, "StartTextDraggingPos"=w739:T15)
                n301 = case shown="False" w737 {
                  tunnel: w736 -> [w745 w770]
                  tunnel: [w744 w769] -> w735
                  tunnel: w733 -> [w741 w765]
                  tunnel: w734 -> [w740 _]
                  tunnel: [w743 "UpdateIcon:2" ("y")] -> w732
                  tunnel: w738 -> [w746 _]
                  tunnel: w739 -> [w742 _]
                  frame False {
                    n302 = case shown="True" w746 {
                      tunnel: w745 -> [w748 w762]
                      tunnel: [w748 w761] -> w744
                      tunnel: ["Idle" "Generate icon"] -> w743
                      tunnel: w742 -> [_ w758]
                      tunnel: w741 -> [_ w759]
                      tunnel: w740 -> [_ w757]
                      frame False {
                      }
                      frame True {
                        n303 = Subtract(x=w759, y=w758) -> (x-y=w754:T15)
                        n304 = Unbundle By Name(w757) -> ("Offset.X"=w752:i32, "Offset.Y"=w751:i32)
                        n305 = Divide(x=w754, y=u8 4 ("f")) -> (x/y=w753:cluster{"Horizontal":dbl, "Vertical":dbl})
                        n306 = Unbundle By Name(w753) -> ("Horizontal"=w750:dbl, "Vertical"=w749:dbl)
                        n307 = Bundle By Name(cluster=w762, "Offset.X"=w752, "Offset.Y"=w751) -> (w756:T18)
                        n308 = Bundle By Name(cluster=w756, "Offset.X"=w750, "Offset.Y"=w749) -> (w761:T18)
                      }
                    }
                  }
                  frame True {
                    w763 = T15 {"Horizontal"=10, "Vertical"=10}  # IconSize
                    n309 = property on="_IconPreview" class="Pict"() -> ("Position"=w773:T30)  [unwired: 2 in, 2 out]
                    n310 = Divide(x=w763, y=2.0 ("Waveform Chart")) -> (x/y=w775:cluster{"Horizontal":dbl, "Vertical":dbl})
                    n311 = Add(x=w773, y=T30 {"Left"=0, "Top"=16}) -> (x+y=w772:T30)
                    n312 = Subtract(x=w765, y=w775) -> (x-y=w764:cluster{"Horizontal":dbl, "Vertical":dbl})
                    n313 = Subtract(x=w764, y=w772) -> (x-y=w767:cluster{dbl, dbl})
                    n314 = Divide(x=w767, y=u8 4 ("Disabled")) -> (x/y=w766:cluster{dbl, dbl})
                    n315 = Bundle By Name(cluster=w770, "BgIconOffset"=w766) -> (w769:T18)
                  }
                }
              }
              event Mouse Up; Mouse Leave {
                n316 = event-data() -> ()  [unwired: 1 in, 1 out]
                n317 = Unbundle By Name(w779) -> ("OverrideMethod"=w778:path)
                n318 = Bundle By Name(cluster=w783, "DraggingText"=FALSE) -> (w782:T18)
              }
              event "_MethodSignature": Value Change {
                n319 = event-data() -> ("OldVal"=w794:u16)  [unwired: 1 in]
                n320 = Unbundle By Name(w795) -> ("Signatures.SignatureText"=w787:string[])  [unwired: 1 out]
                n321 = local read "_MethodDescription"() -> (w790:string)
                n322 = property on="_MethodSignature" class="Ring (strict)"() -> ("Strings []"=w801:string[])  [unwired: 2 in, 2 out]
                n323 = Decrement(x=w794) -> (x-1=w786:u16)
                n324 = Index Array(array=w787, index=w786) -> (element=w793:string)
                n325 = Greater Than 0?(x=w794) -> (x > 0?=w788:bool)
                n326 = Array Size(array=w801) -> (size(s)=w800:i32)
                n327 = call <resource>:"UpdateMethodSignatureText.vi"("TagCodedStringIn"=w793) -> ("StringOut"=w792:string)  [unwired: 10 in]
                n328 = Decrement(x=w800) -> (x-1=w799:i32)
                n329 = String Length(string=w792) -> (length=w791:i32)
                n330 = String Length(string=w790) -> (length=w789:i32)
                n331 = Equal?(x="_MethodSignature", y=w799) -> (x = y?=w798:bool)
                n332 = case shown="False" w798 {
                  tunnel: ["Idle" w832] -> w797
                  tunnel: "_MethodSignature" -> [w817 _]
                  tunnel: w791 -> [w815 _]
                  tunnel: w790 -> [w810 _]
                  tunnel: w789 -> [w816 _]
                  tunnel: w788 -> [w813 _]
                  tunnel: w787 -> [w811 _]
                  frame False {
                    n333 = Subtract(x=w816, y=w815) -> (x-y=w814:i32)
                    n334 = String Subset(string=w810, length (rest)=w814) -> (substring=w812:string)  [unwired: 1 in]
                    n335 = Select(t=w812, s=w813, f=w810) -> (s? t:f=w809:string)
                    n336 = String To Byte Array(string=w809) -> (unsigned byte array=w808:u8[])
                    n337 = Delete From Array(array=w808) -> (deleted portion=w807:u8)  [unwired: 2 in, 1 out]
                    n338 = Greater?(x=w807, y=u8 32) -> (0:w805:bool)
                    n339 = Select(t="\r", s=w805, f="") -> (s? t:f=w804:string)
                    n340 = case shown="0" w817 {
                      selector: w817 -> [w826 _]
                      tunnel: w811 -> [w825 _]
                      tunnel: w809 -> [w820 w828]
                      tunnel: w804 -> [w819 w827]
                      frame 1.., Default {
                        n341 = Decrement(x=w826) -> (x-1=w821:u16)
                        n342 = Index Array(array=w825, index=w821) -> (element=w824:string)
                        n343 = call <resource>:"UpdateMethodSignatureText.vi"("TagCodedStringIn"=w824) -> ("StringOut"=w823:string)  [unwired: 10 in]
                        n344 = Concatenate Strings(w820, w819, w823) -> (w822:string)
                        n345 = local write "_MethodDescription"(w822) -> ()
                      }
                      frame 0 {
                        n346 = Concatenate Strings(w828, w827) -> (w829:string)
                        n347 = local write "_MethodDescription"(w829) -> ()
                      }
                    }
                  }
                  frame True {
                    n348 = local write "_MethodSignature"(0) -> ()
                    n349 = call <resource>:"MethodSignatureDialogvi.vi"() -> ("Cancelled"=w831:bool)  [unwired: 11 in]
                    n350 = case shown="True" w831 {
                      tunnel: ["UpdateMethodSignatures" "Idle"] -> w832
                      frame False {
                      }
                      frame True {
                      }
                    }
                  }
                }
              }
              event "_Cancel": Value Change {
                n351 = event-data() -> ()  [unwired: 1 in, 2 out]
              }
              event Panel Close? {
                w841 = TRUE
                n352 = event-data() -> ()  [unwired: 1 in, 4 out]
                n353 = event-data("Discard?"=w841) -> ()  [unwired: 1 in, 1 out]
              }
              event "_CreateMethod", "_CreateOpenClass": Value Change {
                w847 = 2 ("y")
                n354 = event-data() -> ()  [unwired: 1 in, 2 out]
                n355 = local read "_Method"() -> (w853:i32[])
                n356 = local read "_Property"() -> (w850:string[])
                n357 = Array Size(array=w853) -> (size(s)=w849:i32)
                n358 = Array Size(array=w850) -> (size(s)=w848:i32)
                n359 = Greater Or Equal?(x=w849, y=w847) -> (x >= y?=w846:bool)
                n360 = Greater Or Equal?(x=w848, y=w847) -> (x >= y?=w845:bool)
                n361 = Or(x=w846, y=w845) -> (x .or. y?=w844:bool)
                n362 = case shown="True" w844 {
                  tunnel: ["Exit" "CreateMethodIcons"] -> w851
                  frame False {
                  }
                  frame True {
                    (unwired) "UpdateIcon:Quit"
                  }
                }
              }
              event "_Property": Value Change {
                n363 = event-data() -> ()  [unwired: 1 in, 1 out]
                n364 = local read "PropertyNodeMethodNaming"() -> (w859:enum16{"Read/Write Naming", "Get/Set Naming"})
                n365 = local read "_MethodType"() -> (w865:T2)
                n366 = property on="_Method" class="LstBox (strict)"() -> ("Item Names"=w866:string[])  [unwired: 2 in, 2 out]
                n367 = local read "_Method"() -> (w868:i32[])
                n368 = call <resource>:"BaseProvider_IniFileSettings.vi"() -> ("IniFileSettings"=w862:T34)  [unwired: 18 in, 1 out]
                n369 = Unbundle By Name(w862) -> ("FileNamingOption"=w861:T35)
                n370 = Empty String/Path?(string/path="_Property") -> (empty?=w874:bool[])
                n371 = Index Array(array=w868) -> (element=w872:i32)  [unwired: 1 in]
                n372 = Equal?(x="_Property", y="ClassAttribute" ("Left Cell String(Main name)")) -> (x = y?=w875:bool[])
                n373 = Equal?(x="_Property", y="ObjectAttribute" ("Left Cell String(Main name)")) -> (x = y?=w876:bool[])
                n374 = Equal?(x=w859, y=enum16{"Read/Write Naming", "Get/Set Naming"}."Read/Write Naming") -> (x = y?=w857:bool)
                n375 = Equal?(x=w865, y=T2."Property Node") -> (x = y?=w860:bool)
                n376 = Compound Arithmetic op=OR(w876, w875, w874) -> (w873:bool[])
                n377 = Index Array(array=w866, index=w872) -> (element=w880:string)
                n378 = Or Array Elements(Boolean array=w873) -> (logical OR=w871:bool)
                n379 = case shown="False" w871 {
                  tunnel: w880 -> [w890 _]
                  tunnel: [w889 "UpdateIcon"] -> w879
                  tunnel: w870 -> [w888 w922]
                  tunnel: [w887 w921] -> w869
                  tunnel: w868 -> [w886 _]
                  tunnel: "_Property" -> [w885 _]
                  tunnel: w866 -> [w884 _]
                  tunnel: w860 -> [w883 _]
                  tunnel: w861 -> [w882 _]
                  tunnel: w857 -> [w881 _]
                  frame False {
                    n380 = case shown="Default" w890 {
                      tunnel: ["UpdateIcon" "Idle"] -> w889
                      tunnel: w888 -> [w904 w919]
                      tunnel: [w903 w918] -> w887
                      tunnel: w886 -> [w901 _]
                      tunnel: w885 -> [w895 _]
                      tunnel: w884 -> [w900 _]
                      tunnel: w883 -> [w893 _]
                      tunnel: w882 -> [w896 _]
                      tunnel: w881 -> [w891 _]
                      frame Default {
                        n381 = Compound Arithmetic op=AND(w891, w893) -> (w892:bool)
                        n382 = call <resource>:"CreateMethodNames.vi"("_Method"=w901, "FileNamingOption"=w896, "_Property"=w895, "Item Names"=w900, "Use Read/Write"=w892) -> ("MethodNames"=w902:string[], "Attribute/PropertyNames"=w897:string[])
                        n383 = for {
                          tunnel: w895 -> [w910] mode=indexing
                          tunnel: [w907] -> w894
                          stop <- w907 stop-if-true
                          n384 = Match Pattern(string=w910, regular expression="^ClassAttribute" ("Left Cell String(Main name)")) -> (offset past match=w908:i32)  [unwired: 1 in, 3 out]
                          n385 = Greater Or Equal To 0?(x=w908) -> (x >= 0?=w907:bool)
                        }
                        n386 = Index Array(array=w902) -> (element=w899:string)  [unwired: 1 in]
                        n387 = case shown="True" w893 {
                          tunnel: w899 -> [w911 _]
                          tunnel: [w911 w912] -> w898
                          tunnel: w897 -> [_ w916]
                          frame False {
                          }
                          frame True {
                            n388 = Array To Spreadsheet String(delimiter (Tab)="/", array=w916, 3:"%s" ("format string")) -> (spreadsheet string=w913:string)
                            n389 = call <vilib>:"Trim Whitespace.vi"("string"=w913) -> ("trimmed string"=w912:string)  [unwired: 1 in]
                          }
                        }
                        n390 = local write "_MethodIconName"(w899) -> ()
                        n391 = Bundle By Name(cluster=w904, "MethodNames"=w902) -> (w903:T18)
                        n392 = local write "_MethodName"(w898) -> ()
                        n393 = case shown="True" w894 {
                          frame False {
                          }
                          frame True {
                            n394 = local write "_DynamicDispatch"(FALSE ("_DynamicDispatch")) -> ()
                          }
                        }
                      }
                      frame "" {
                        n395 = Bundle By Name(cluster=w919, "MethodNames"=string[] []) -> (w918:T18)
                      }
                    }
                  }
                  frame True {
                    w924 = "" ("Method Name")
                    n396 = local write "_MethodName"(w924) -> ()
                    n397 = local write "_MethodIconName"(w924) -> ()
                    n398 = Bundle By Name(cluster=w922, "MethodNames"=string[] []) -> (w921:T18)
                  }
                }
              }
              event "_OverrideMethods": Value Change {
                n399 = event-data() -> ()  [unwired: 1 in, 4 out]
                n400 = local read "_OverrideMethods"() -> (w927:i32)
                n401 = Unbundle By Name(w939) -> ("OverrideScope"=w941:T33, "AllOverrideMethods"=w943:path[], "OverrideMethodsIdx"=w928:i32[])
                n402 = Unbundle By Name(w939) -> ("ColorProtected"=w938:u32, "ColorPrivate"=w937:u32, "ColorPublic"=w936:u32)
                n403 = Index Array(array=w928, index=w927) -> (element=w926:i32)
                n404 = Index Array(array=w943, index=w926) -> (element=w930:path)
                n405 = Index Array(array=w941, index=w926) -> (element=w940:T22)
                n406 = case shown="\"invalid scope\", Default" w940 {
                  tunnel: [w944 w945 w946] -> w933
                  tunnel: w938 -> [_ w945 _]
                  tunnel: w936 -> [w944 _ _]
                  tunnel: w937 -> [_ _ w946]
                  frame "invalid scope", Default {
                  }
                  frame "protected" {
                  }
                  frame "private" {
                  }
                }
                n407 = call <vilib>:"Get File Extension.vi"("file"=w930) -> ("filename without extension"=w929:string)  [unwired: 6 in, 4 out]
                n408 = local read "_BodyBk"() -> (w934:T1)
                n409 = local write "_MethodName"(w929) -> ()
                n410 = local write "_MethodIconName"(w929) -> ()
                n411 = Bundle(cluster=w934, "Color"=w933) -> (w935:T1)  [unwired: 1 in]
                n412 = call <vilib>:"Set Busy.vi"() -> ()  [unwired: 10 in, 2 out]
                n413 = local write "_BodyBk"(w935) -> ()
              }
              event "Filter": Value Change {
                n414 = event-data() -> ()  [unwired: 1 in, 6 out]
                n415 = Unbundle By Name(w958) -> ("OverrideMethodsNames"=w953:string[])
                n416 = call <vilib>:"Trim Whitespace.vi"("string"="Filter") -> ("trimmed string"=w951:string)  [unwired: 1 in]
                n417 = Empty String/Path?(string/path=w951) -> (empty?=w949:bool)
                n418 = Equal?(x=w951, y="Filter name" ("InterfaceFilter")) -> (x = y?=w948:bool)
                n419 = Or(x=w949, y=w948) -> (x .or. y?=w947:bool)
                n420 = for {
                  tunnel: w953 -> [w967] mode=indexing
                  tunnel: w951 -> [w970]
                  tunnel: [w967] -> w952 mode=indexing if=w965
                  tunnel: [w966] -> w955 mode=indexing if=w965
                  tunnel: w947 -> [w964]
                  i -> [w966]
                  n421 = To Lower Case(string=w970) -> (all lower case string=w962:string)
                  n422 = To Lower Case(string=w967) -> (all lower case string=w963:string)
                  n423 = Match Pattern(string=w963, regular expression=w962) -> (offset past match=w969:i32)  [unwired: 1 in, 3 out]
                  n424 = Greater Or Equal To 0?(x=w969) -> (x >= 0?=w968:bool)
                  n425 = Or(x=w968, y=w964) -> (x .or. y?=w965:bool)
                }
                n426 = Bundle By Name(cluster=w961, "OverrideMethodsIdx"=w955) -> (w957:T18)
                n427 = property on="_OverrideMethods" class="LstBox (strict)"("Item Names"=w952, "Top Row"=0) -> ()  [unwired: 2 in, 2 out]
              }
              event "_AddFolder": Value Change {
                n428 = event-data() -> ()  [unwired: 1 in, 6 out]
                n429 = call <resource>:"NewFolderDialog.vi"("error in"=w976, "ClassItemRefIn"=w975) -> ("error out"=w977:errorcluster, "FolderNameOut"=w973:string, "FolderSourceScope"=w972:T22, "Cancelled"=w978:bool, "FolderPath"=w971:path)  [unwired: 5 in]
                n430 = case shown="False" w978 {
                  tunnel: w980 -> [w992 w1007]
                  tunnel: [w993 w1007] -> w979
                  tunnel: [w986 _] -> w974
                  tunnel: w973 -> [w982 _]
                  tunnel: w972 -> [w988 _]
                  tunnel: w971 -> [w987 _]
                  frame False {
                    n431 = Unbundle By Name(w992) -> ("FolderNames"=w983:string[], "FolderPath"=w990:path[], "FolderType"=w989:T33)
                    n432 = Search 1D Array(1D array=w983, element=w982) -> (index of element=w981:i32)  [unwired: 1 in]
                    n433 = case shown="-1" w981 {
                      tunnel: [w996 w1006] -> w991
                      tunnel: w990 -> [w995 w1005]
                      tunnel: [w995 w1004] -> w984
                      tunnel: w989 -> [w994 w1003]
                      tunnel: [w994 w1002] -> w985
                      tunnel: w988 -> [_ w1001]
                      tunnel: w987 -> [_ w1000]
                      tunnel: w982 -> [_ w999]
                      tunnel: w983 -> [w996 w998]
                      tunnel: [_ "UpdateScopeList\nIdle"] -> w986
                      frame 0, Default {
                      }
                      frame -1 {
                        n434 = Build Array (concatenate)(w998, w999) -> (w1006:string[])
                        n435 = Build Array (concatenate)(w1005, w1000) -> (w1004:path[])
                        n436 = Build Array (concatenate)(w1003, w1001) -> (w1002:T33)
                      }
                    }
                    n437 = Bundle By Name(cluster=w992, "FolderNames"=w991, "FolderPath"=w984, "FolderType"=w985) -> (w993:T18)
                  }
                  frame True {
                  }
                }
              }
              event "_MethodDescription": Value Change {
                n438 = event-data() -> ()  [unwired: 1 in, 2 out]
              }
              event "_MethodName": Value Change {
                w1031 = TRUE ("ignore case? (F)")
                n439 = event-data() -> ()  [unwired: 1 in, 2 out]
                n440 = Unbundle By Name(w1039) -> ("ClassName"=w1022:string)
                n441 = local read "_MethodType"() -> (w1018:T2)
                n442 = case shown="Default" w1018 {
                  tunnel: [w1045 w1047] -> w1033
                  tunnel: "_MethodName" -> [w1045 w1046]
                  frame "Property Node" {
                  }
                  frame Default {
                    n443 = call <resource>:"GOOP300_RemoveUnwantedChars.vi"("StringIn"=w1046) -> ("StringOut"=w1047:string)  [unwired: 10 in]
                  }
                }
                n444 = Concatenate Strings(w1022, "[_ ]*" ("string")) -> (w1027:string)
                n445 = Match Pattern(string=w1033, regular expression="\\2E[Vv][Ii][Mm]*") -> (before substring=w1021:string, match substring=w1015:string)  [unwired: 1 in, 2 out]
                n446 = Concatenate Strings("^" ("string"), w1027) -> (w1030:string)
                n447 = Concatenate Strings(w1027, "$" ("string")) -> (w1026:string)
                n448 = To Lower Case(string=w1015) -> (all lower case string=w1014:string)
                n449 = xnode "Match Regular Expression"("input string"=w1021, "regular expression"=w1030, "ignore case? (F)"=w1031) -> ("before match"=w1036:string, "after match"=w1035:string)  [unwired: 3 in, 3 out]
                n450 = Concatenate Strings(w1036, w1035) -> (w1032:string)
                n451 = Match Pattern(string=w1014, regular expression="vim") -> (offset past match=w1012:i32)  [unwired: 1 in, 3 out]
                n452 = Greater Or Equal To 0?(x=w1012) -> (x >= 0?=w1011:bool)
                n453 = xnode "Match Regular Expression"("input string"=w1032, "regular expression"=w1026, "ignore case? (F)"=w1031) -> ("before match"=w1025:string, "after match"=w1024:string)  [unwired: 3 in, 3 out]
                n454 = case shown="True" w1011 {
                  tunnel: w1021 -> [_ w1040]
                  frame False {
                  }
                  frame True {
                    n455 = local write "_MethodName"(w1040) -> ()
                  }
                }
                n456 = property on=".vim" class="Bool (strict)"("Visible"=w1011, "Value"=w1011) -> ()  [unwired: 2 in, 2 out]
                n457 = Concatenate Strings(w1025, w1024) -> (w1017:string)
                n458 = case shown="\"Property Node\"" w1018 {
                  tunnel: w1017 -> [w1041 w1044]
                  tunnel: [w1041 w1042] -> _
                  frame Default {
                    n459 = local write "_MethodIconName"(w1041) -> ()
                  }
                  frame "Property Node" {
                    n460 = Match Pattern(string=w1044, regular expression="/") -> (before substring=w1042:string)  [unwired: 1 in, 3 out]
                  }
                }
                n461 = case shown="\"Property Node\"" w1018 {
                  tunnel: w1020 -> [w1048 w1051]
                  tunnel: [w1048 w1050] -> w1019
                  frame "Property Node" {
                  }
                  frame Default {
                    n462 = Bundle By Name(cluster=w1051, "MethodNames"=string[] []) -> (w1050:T18)
                  }
                }
              }
              event "_DynamicDispatch", "_MustOverride", "_MustCallParent": Value Change {
                n463 = event-data() -> ()  [unwired: 1 in, 6 out]
                n464 = call <resource>:"BaseProvider_IniFileSettings.vi"() -> ("IniFileSettings"=w1276:T34)  [unwired: 18 in, 1 out]
                n465 = Bundle By Name(cluster=w1276, "DynamicDispatchStartValue"="_DynamicDispatch") -> (w1277:T34)
                n466 = call <resource>:"BaseProvider_IniFileSettings.vi"("IniFileSettings"=w1277, "Action"=enum16{"Read", "Load", "Save"}."Save") -> ()  [unwired: 16 in, 2 out]
              }
              event "_MethodIconName": Value Change {
                n467 = event-data() -> ()  [unwired: 1 in, 6 out]
              }
              event "_IconPreview": Mouse Down {
                w1302 = 4 ("y")
                n468 = event-data() -> ("Coords"=w1287:T15)  [unwired: 1 in]
                n469 = property on="_IconPreview" class="Pict"() -> ("Mouse"=w1291:T41)  [unwired: 2 in, 2 out]
                n470 = Unbundle By Name(w1286) -> ("IconDropped"=w1285:i32, "TextBounds"=w1293:T42)
                n471 = Unbundle(w1293) -> ("FirstRow"=w1295:i32, "FirstColumn"=w1296:i32, "LastRow"=w1294:i32, "LastColumn"=w1292:i32)
                n472 = Unbundle By Name(w1291) -> ("Mouse Position.X"=w1301:i32, "Mouse Position.Y"=w1299:i32)
                n473 = Divide(x=w1301, y=w1302) -> (x/y=w1303:dbl)
                n474 = Divide(x=w1299, y=w1302) -> (x/y=w1300:dbl)
                n475 = In Range and Coerce(upper limit=w1294, x=w1300, lower limit=w1295) -> (In Range?=w1297:bool)  [unwired: 1 out]
                n476 = In Range and Coerce(upper limit=w1292, x=w1303, lower limit=w1296) -> (In Range?=w1298:bool)  [unwired: 1 out]
                n477 = And(x=w1297, y=w1298) -> (x .and. y?=w1290:bool)
                n478 = case shown="False" w1290 {
                  tunnel: w1289 -> [w1306 w1332]
                  tunnel: [w1305 w1331] -> w1288
                  tunnel: w1287 -> [w1308 w1330]
                  tunnel: w1286 -> [_ w1329]
                  tunnel: w1285 -> [w1307 _]
                  tunnel: [w1304 "Idle"] -> w1284
                  frame False {
                    n479 = case shown="0.." w1307 {
                      selector: w1307 -> [_ w1313]
                      tunnel: w1306 -> [w1310 w1326]
                      tunnel: [w1310 w1325] -> w1305
                      tunnel: ["Idle" ("y") "ShowDragIcon:UpdateIcon" ("y")] -> w1304
                      tunnel: w1308 -> [_ w1312]
                      frame Default {
                      }
                      frame 0.. {
                        w1311 = T15 {"Horizontal"=10, "Vertical"=10}  # IconSize
                        n480 = Divide(x=w1311, y=2) -> (x/y=w1322:cluster{"Horizontal":dbl, "Vertical":dbl})
                        n481 = Subtract(x=w1312, y=w1322) -> (x-y=w1316:cluster{"Horizontal":dbl, "Vertical":dbl})
                        n482 = property on="_IconPreview" class="Pict"() -> ("Position"=w1320:T30)  [unwired: 2 in, 2 out]
                        n483 = Add(x=w1320, y=T30 {"Left"=0, "Top"=16}) -> (x+y=w1319:T30)
                        n484 = Subtract(x=w1316, y=w1319) -> (x-y=w1317:cluster{dbl, dbl})
                        n485 = Divide(x=w1317, y=u8 4 ("Disabled")) -> (x/y=w1315:cluster{dbl, dbl})
                        n486 = Bundle By Name(cluster=w1326, "IconSelected"=w1313, "DraggingIcon"=TRUE ("Draging"), "BgIconOffset"=w1315) -> (w1325:T18)
                      }
                    }
                  }
                  frame True {
                    n487 = Unbundle By Name(w1329) -> ("Offset.X"=w1334:i32, "Offset.Y"=w1335:i32)
                    n488 = Bundle("X"=w1334, "Y"=w1335) -> (w1338:cluster{"X":i32, "Y":i32})  [unwired: 1 in]
                    n489 = Multiply(x=w1338, y=4) -> (x*y=w1339:cluster{"X":i32, "Y":i32})
                    n490 = Subtract(x=w1330, y=w1339) -> (x-y=w1337:T15)
                    n491 = Bundle By Name(cluster=w1332, "DraggingIcon"=FALSE, "DraggingText"=TRUE, "StartTextDraggingPos"=w1337) -> (w1331:T18)
                  }
                }
              }
              event "_IconPreview": Mouse Up {
                w1343 = FALSE ("DraggingText")
                n492 = event-data() -> ()  [unwired: 1 in, 3 out]
                n493 = Unbundle By Name(w1342) -> ("IconSelected"=w1341:i32)
                n494 = Bundle By Name(cluster=w1346, "IconDropped"=w1341, "DraggingText"=w1343, "DraggingIcon"=w1343, "Moving"=w1343) -> (w1345:T18)
              }
              event "_IconPreview": Mouse Leave {
                n495 = event-data() -> ()  [unwired: 1 in, 1 out]
                n496 = Unbundle By Name(w1349) -> ("OverrideMethod"=w1348:path)
                n497 = Bundle By Name(cluster=w1352, "DraggingText"=FALSE) -> (w1351:T18)
              }
              event "_IconPreview": Mouse Move {
                n498 = event-data() -> ("Coords"=w1360:T15)  [unwired: 1 in]
                n499 = Unbundle By Name(w1356) -> ("DraggingText"=w1362:bool)
                n500 = Unbundle By Name(w1356) -> ("OverrideMethod"=w1355:path)
                n501 = Unbundle By Name(w1356) -> ("StartTextDraggingPos"=w1361:T15)
                n502 = case shown="False" w1362 {
                  tunnel: w1359 -> [w1364 w1378]
                  tunnel: [w1364 w1377] -> w1358
                  tunnel: ["Idle" "UpdateIcon"] -> w1357
                  tunnel: w1361 -> [_ w1374]
                  tunnel: w1360 -> [_ w1375]
                  tunnel: w1356 -> [_ w1373]
                  frame False {
                  }
                  frame True {
                    n503 = Subtract(x=w1375, y=w1374) -> (x-y=w1370:T15)
                    n504 = Unbundle By Name(w1373) -> ("Offset.X"=w1368:i32, "Offset.Y"=w1367:i32)
                    n505 = Divide(x=w1370, y=u8 4 ("f")) -> (x/y=w1369:cluster{"Horizontal":dbl, "Vertical":dbl})
                    n506 = Unbundle By Name(w1369) -> ("Horizontal"=w1366:dbl, "Vertical"=w1365:dbl)
                    n507 = Bundle By Name(cluster=w1378, "OldOffset.X"=w1368, "OldOffset.Y"=w1367) -> (w1372:T18)
                    n508 = Bundle By Name(cluster=w1372, "Offset.X"=w1366, "Offset.Y"=w1365) -> (w1377:T18)
                  }
                }
              }
              event "_IconPreview": Mouse Enter {
                n509 = event-data() -> ()  [unwired: 1 in, 1 out]
                n510 = Unbundle By Name(w1381) -> ("OverrideMethod"=w1380:path)
                n511 = Unbundle By Name(w1381) -> ("DraggingIcon"=w1386:bool, "IconDropped"=w1385:i32)
                n512 = case shown="True" w1386 {
                  tunnel: w1384 -> [w1389 w1390]
                  tunnel: [w1388 w1390] -> w1383
                  tunnel: w1385 -> [w1387 _]
                  frame False {
                    n513 = Bundle By Name(cluster=w1389, "IconSelected"=w1387) -> (w1388:T18)
                  }
                  frame True {
                  }
                }
              }
              event "_IconSize", "_TextAlignment": Value Change {
                n514 = event-data() -> ()  [unwired: 1 in, 6 out]
                n515 = Bundle By Name(cluster=w1395, "Offset"=cluster{"X":i32, "Y":i32} {"X"=0, "Y"=0}) -> (w1393:T18)
              }
              event "_MethodLocation": Value Change {
                (unwired) T19."Disabled and Grayed Out" ("Disabled")
                n516 = event-data() -> ()  [unwired: 1 in, 2 out]
                n517 = Unbundle By Name(w1397) -> ("ColorPublic"=w1410:u32, "ColorPrivate"=w1409:u32, "ColorProtected"=w1408:u32, "AF"=w1400:bool)
                n518 = Unbundle By Name(w1397) -> ("FolderType"=w1415:T33)
                n519 = Index Array(array=w1415, index="_MethodLocation") -> (element=w1413:T22)
                n520 = case shown="\"protected\"" w1413 {
                  tunnel: [T19."Enabled" ("Disabled") T19."Disabled and Grayed Out" ("Disabled") T19."Disabled and Grayed Out" ("Disabled") T19."Disabled and Grayed Out" ("Disabled") T19."Disabled and Grayed Out" ("Disabled")] -> w1412
                  tunnel: [T7."Public" ("_Visibility") T7."Public" ("_Visibility") T7."Community" ("_Visibility") T7."Private" ("_Visibility") T7."Protected" ("_Visibility")] -> w1411
                  tunnel: w1410 -> [w1426 w1433 w1438 _ _]
                  tunnel: [w1426 w1433 w1438 w1443 w1450] -> w1405
                  tunnel: w1409 -> [_ _ _ w1443 _]
                  tunnel: w1408 -> [_ _ _ _ w1450]
                  tunnel: [TRUE TRUE FALSE FALSE FALSE] -> w1399
                  tunnel: [T19."Enabled" ("Disabled") T19."Enabled" ("Disabled") T19."Disabled and Grayed Out" ("Disabled") T19."Disabled and Grayed Out" ("Disabled") T19."Disabled and Grayed Out" ("Disabled")] -> w1398
                  frame "invalid scope", Default {
                  }
                  frame "public" {
                    n521 = call <resource>:"BaseProvider_IniFileSettings.vi"() -> ("IniFileSettings"=w1428:T34)  [unwired: 18 in, 1 out]
                    n522 = Unbundle By Name(w1428) -> ("DynamicDispatchStartValue"=w1427:bool)
                    n523 = local write "_DynamicDispatch"(w1427) -> ()
                  }
                  frame "community" {
                  }
                  frame "private" {
                  }
                  frame "protected" {
                    n524 = call <resource>:"BaseProvider_IniFileSettings.vi"() -> ("IniFileSettings"=w1445:T34)  [unwired: 18 in, 1 out]
                    n525 = Unbundle By Name(w1445) -> ("DynamicDispatchStartValue"=w1444:bool)
                    n526 = local write "_DynamicDispatch"(w1444) -> ()
                  }
                }
                n527 = local read "_MethodType"() -> (w1401:T2)
                n528 = case shown="Default" w1401 {
                  tunnel: w1398 -> [w1418 _]
                  tunnel: w1399 -> [w1417 _]
                  tunnel: [w1418 T19."Disabled and Grayed Out" ("Disabled")] -> w1403
                  tunnel: [w1417 _] -> w1402
                  frame Default {
                  }
                  frame "Override Method" {
                  }
                }
                n529 = local read "_BodyBk"() -> (w1406:T1)
                n530 = property on="_Visibility" class="RadioBtnsControl (strict)"("Disabled"=w1412) -> ()  [unwired: 2 in, 2 out]
                n531 = Bundle(cluster=w1406, "Color"=w1405) -> (w1407:T1)  [unwired: 1 in]
                n532 = local write "_Visibility"(w1411) -> ()
                n533 = case shown="True" w1400 {
                  tunnel: w1402 -> [_ w1421]
                  tunnel: w1403 -> [_ w1420]
                  frame False {
                  }
                  frame True {
                    n534 = property on="_AddMessageClass" class="Bool (strict)"("DisabledEnum"=w1420, "Value"=w1421) -> ()  [unwired: 2 in, 2 out]
                  }
                }
                n535 = local write "_BodyBk"(w1407) -> ()
              }
              event "_FontCompression", "_CapitalOnly": Value Change {
                n536 = event-data() -> ()  [unwired: 1 in, 2 out]
              }
              event Value Change {
                n537 = event-data() -> ()  [unwired: 1 in, 6 out]
                n538 = Unbundle By Name(w1459) -> ("OverrideMethod"=w1455:path)
                n539 = Empty String/Path?(string/path=w1455) -> (empty?=w1458:bool)
                n540 = Select(t="UpdateIcon", s=w1458, f="UpdateIconFromParentMethod") -> (s? t:f=w1460:string)
              }
              event "_Visibility": Value Change {
                (unwired) T7."Community" ("_Visibility")
                n541 = event-data() -> ()  [unwired: 1 in, 2 out]
                n542 = Unbundle By Name(w1463) -> ("ColorProtected"=w1476:u32, "ColorPrivate"=w1474:u32, "ColorPublic"=w1475:u32, "AF"=w1464:bool)
                n543 = case shown="\"Private\"" "_Visibility" {
                  tunnel: [w1488 w1493 w1496 w1499] -> w1472
                  tunnel: w1476 -> [_ w1493 _ _]
                  tunnel: w1475 -> [w1488 _ _ w1499]
                  tunnel: w1474 -> [_ _ w1496 _]
                  tunnel: [T19."Enabled" ("Disabled") T19."Disabled and Grayed Out" ("Disabled") T19."Disabled and Grayed Out" ("Disabled") T19."Disabled and Grayed Out" ("Disabled")] -> w1469
                  tunnel: [TRUE FALSE FALSE FALSE] -> w1468
                  frame "Public", Default {
                    n544 = call <resource>:"BaseProvider_IniFileSettings.vi"() -> ("IniFileSettings"=w1485:T34)  [unwired: 18 in, 1 out]
                    n545 = Unbundle By Name(w1485) -> ("DynamicDispatchStartValue"=w1484:bool)
                    n546 = local write "_DynamicDispatch"(w1484) -> ()
                  }
                  frame "Protected" {
                    n547 = call <resource>:"BaseProvider_IniFileSettings.vi"() -> ("IniFileSettings"=w1490:T34)  [unwired: 18 in, 1 out]
                    n548 = Unbundle By Name(w1490) -> ("DynamicDispatchStartValue"=w1489:bool)
                    n549 = local write "_DynamicDispatch"(w1489) -> ()
                  }
                  frame "Private" {
                  }
                  frame "Community" {
                  }
                }
                n550 = local read "_MethodType"() -> (w1465:T2)
                n551 = case shown="Default" w1465 {
                  tunnel: w1469 -> [w1480 _]
                  tunnel: w1468 -> [w1479 _]
                  tunnel: [w1480 T19."Disabled and Grayed Out" ("Disabled")] -> w1467
                  tunnel: [w1479 _] -> w1466
                  frame Default {
                  }
                  frame "Override Method" {
                  }
                }
                n552 = local read "_BodyBk"() -> (w1471:T1)
                n553 = Bundle(cluster=w1471, "Color"=w1472) -> (w1473:T1)  [unwired: 1 in]
                n554 = local write "_BodyBk"(w1473) -> ()
                n555 = case shown="True" w1464 {
                  tunnel: w1466 -> [_ w1483]
                  tunnel: w1467 -> [_ w1482]
                  frame False {
                  }
                  frame True {
                    n556 = property on="_AddMessageClass" class="Bool (strict)"("DisabledEnum"=w1482, "Value"=w1483) -> ()  [unwired: 2 in, 2 out]
                  }
                }
              }
              event Mouse Enter; Mouse Leave {
                n557 = event-data() -> ("Type"=w1507:T24, "CtlRef"=w1512:refnum<vi>)  [unwired: 1 in, 1 out]
                n558 = Unbundle By Name(w1502) -> ("OverrideMethod"=w1501:path)
                n559 = Equal?(x=w1507, y=lveventtype."Mouse Enter") -> (x = y?=w1505:bool)
                n560 = property class="Clust (strict)"(reference=w1512) -> (reference out=w1511:refnum<vi>, error out=w1510:errorcluster, "Value"=w1509:T43)  [unwired: 1 in]
                n561 = Bundle By Name(cluster=w1509, "Decal"=w1505) -> (w1508:T43)
                n562 = property class="Clust (strict)"(reference=w1511, error in=w1510, "Value"=w1508) -> ()  [unwired: 2 out]
              }
              event "_MethodType": Value Change {
                (unwired) T23 {"Left"=329, "Top"=250, "Right"=1087, "Bottom"=690} ("Front Panel Window:Panel Bounds")
                # "width = 1108"
                n563 = local read "PropertyNodeMethodNaming"() -> (w1515:enum16{"Read/Write Naming", "Get/Set Naming"})
                n564 = event-data() -> ("OldVal"=w1530:T2, "NewVal"=w1528:T2)  [unwired: 1 in]
                n565 = Unbundle By Name(w1540) -> ("AF"=w1539:bool, "MethodCaptionName"=w1527:string, "MethodLocation"=w1529:string[][])
                n566 = local read "_Method"() -> (w1518:i32[])
                n567 = case shown="\"Property Node\"" w1530 {
                  tunnel: w1529 -> [_ w1566]
                  frame Default {
                  }
                  frame "Property Node" {
                    n568 = property on="_MethodLocation" class="MCListbox (strict)"("ItemNames"=w1566, "Value"=0 ("_MethodLocation")) -> ()  [unwired: 2 in, 2 out]
                  }
                }
                n569 = Equal?(x=w1515, y=enum16{"Read/Write Naming", "Get/Set Naming"}."Get/Set Naming") -> (x = y?=w1513:bool)
                n570 = local read "_Visibility"() -> (w1538:T7)
                n571 = case shown="\"Property Node\"" "_MethodType" {
                  tunnel: [w1590 w1602 w1611 w1625] -> w1548
                  tunnel: T23 {"Left"=329, "Top"=250, "Right"=1437, "Bottom"=775} ("Front Panel Window:Panel Bounds") -> [_ w1602 w1611 w1625]
                  tunnel: T23 {"Left"=329, "Top"=250, "Right"=1119, "Bottom"=775} ("Front Panel Window:Panel Bounds") -> [w1590 _ _ _]
                  tunnel: ["UpdateMethodSettings\nIdle" "UpdateMethodSettings\nUpdateOverRideMethods" "UpdateMethodSettings\nUpdateProperties" "UpdateMethodSettings\nUpdateProperties"] -> w1560
                  tunnel: w1540 -> [w1588 w1600 w1609 w1623]
                  tunnel: [w1586 w1596 w1607 w1613] -> w1547
                  tunnel: [_ u8 2 ("Disabled") _ _] -> w1546
                  tunnel: [_ TRUE _ _] -> w1545
                  tunnel: [1 ("Selection Mode") 1 ("Selection Mode") 3 ("Selection Mode") 3 ("Selection Mode")] -> w1544
                  tunnel: [TRUE ("LimitToSpecificProviderTypeOfSameType(True)") FALSE ("LimitToSpecificProviderTypeOfSameType(True)") TRUE ("LimitToSpecificProviderTypeOfSameType(True)") TRUE ("LimitToSpecificProviderTypeOfSameType(True)")] -> w1534
                  tunnel: [T19."Enabled" ("Disabled") T19."Disabled and Grayed Out" ("Disabled") T19."Enabled" ("Disabled") T19."Enabled" ("Disabled")] -> w1535
                  tunnel: [w1582 _ FALSE FALSE] -> w1531
                  tunnel: w1518 -> [w1581 w1591 _ _]
                  tunnel: [_ _ _ TRUE] -> w1516
                  tunnel: w1513 -> [_ _ _ w1612]
                  frame "Normal Method", Default {
                    n572 = local read "_MethodName"() -> (w1583:string)
                    n573 = Index Array(array=w1581) -> (element=w1580:i32)  [unwired: 1 in]
                    n574 = Unbundle By Name(w1588) -> ("AF"=w1582:bool, "NormalMethods"=w1586:T12[])
                    n575 = Build Array(w1580) -> (w1579:i32[])
                    n576 = local write "_Method"(w1579) -> ()
                    n577 = property on="_MethodName" class="Str"("Val(Sgnl)"=w1583) -> ()  [unwired: 2 in, 2 out]
                  }
                  frame "Override Method" {
                    n578 = Index Array(array=w1591) -> (element=w1593:i32)  [unwired: 1 in]
                    n579 = Unbundle By Name(w1600) -> ("OverrideMethods"=w1596:T12[])
                    n580 = Build Array(w1593) -> (w1592:i32[])
                    n581 = local write "_Method"(w1592) -> ()
                  }
                  frame "Property Method" {
                    w1603 = "" ("Method Name")
                    n582 = Unbundle By Name(w1609) -> ("PropertyMethods"=w1607:T12[])
                    n583 = local write "_MethodName"(w1603) -> ()
                    n584 = local write "_MethodIconName"(w1603) -> ()
                  }
                  frame "Property Node" {
                    w1618 = "" ("Method Name")
                    n585 = Unbundle By Name(w1623) -> ("PropertyNodeMethods"=w1614:T12[])
                    n586 = local write "_MethodName"(w1618) -> ()
                    n587 = local write "_MethodIconName"(w1618) -> ()
                    n588 = call <resource>:"RenamePropertyMethods.vi"("RenameToGet/Set"=w1612, "PropertyNodeMethods"=w1614) -> ("Array"=w1613:T12[])  [unwired: 9 in]
                    n589 = property on="_MethodLocation" class="MCListbox (strict)"("ItemNames"=string[][] [["properties", "properties", "<any scope>"]] ("Item Names"), "Value"=0 ("_MethodLocation")) -> ()  [unwired: 2 in, 2 out]
                  }
                }
                n590 = Equal?(x=w1538, y=T7."Public" ("_Visibility")) -> (x = y?=w1536:bool)
                n591 = property on="_MethodName" class="Str"("Disabled"=w1546) -> ()  [unwired: 2 in, 2 out]
                n592 = case shown="False" w1536 {
                  tunnel: w1535 -> [_ w1569]
                  tunnel: w1534 -> [_ w1568]
                  tunnel: [T19."Disabled and Grayed Out" ("Disabled") w1569] -> w1533
                  tunnel: [_ w1568] -> w1532
                  frame False {
                  }
                  frame True {
                  }
                }
                n593 = local write "_AddMessageClass"(w1531) -> ()
                n594 = property class="VI"() -> ("Front Panel.PanelBounds"=w1553:T23)  [unwired: 2 in, 2 out]
                n595 = property on="_MethodsLocationOverrideInfo" class="Str"("Visible"=w1545) -> ()  [unwired: 2 in, 2 out]
                n596 = Unbundle(w1548) -> ("Left"=w1558:i16, "Top"=w1556:i16, "Right"=w1559:i16, "Bottom"=w1557:i16)
                n597 = property on="_Method" class="LstBox (strict)"("Selection Mode"=w1544) -> ()  [unwired: 2 in, 2 out]
                n598 = case shown="\"Property Node\"" w1528 {
                  tunnel: w1527 -> [_ w1564]
                  tunnel: ["Property Name" ("MethodCaptionName") w1564] -> w1526
                  frame "Property Node" {
                  }
                  frame Default {
                  }
                }
                n599 = Unbundle(w1553) -> ("Left"=w1552:i16, "Top"=w1551:i16)  [unwired: 2 out]
                n600 = Subtract(x=w1557, y=w1556) -> (x-y=w1554:i16)
                n601 = Subtract(x=w1559, y=w1558) -> (x-y=w1555:i16)
                n602 = for {
                  tunnel: w1547 -> [w1575] mode=indexing
                  tunnel: [w1576] -> w1520 mode=indexing
                  tunnel: [w1574] -> w1522 mode=indexing
                  tunnel: [w1573] -> w1523 mode=indexing
                  tunnel: [w1572] -> w1517 mode=indexing
                  n603 = Unbundle(w1575) -> ("Name"=w1574:string, "Path"=w1573:path, "DynamicDispatch"=w1572:T14)  [unwired: 3 out]
                  n604 = case shown="Default" w1574 {
                    tunnel: [0 -1] -> w1576
                    frame Default {
                    }
                    frame "" {
                    }
                  }
                }
                n605 = case shown="True" w1539 {
                  tunnel: w1532 -> [_ w1571]
                  tunnel: w1533 -> [_ w1570]
                  frame False {
                  }
                  frame True {
                    n606 = property on="_AddMessageClass" class="Bool (strict)"("DisabledEnum"=w1570, "Value"=w1571) -> ()  [unwired: 2 in, 2 out]
                  }
                }
                n607 = property on="PropertyNodeMethodNaming" class="Enum (strict)"("Visible"=w1516) -> ()  [unwired: 2 in, 2 out]
                n608 = Add(x=w1552, y=w1555) -> (x+y=w1550:i16)
                n609 = Add(x=w1551, y=w1554) -> ()  [unwired: 1 out]
                n610 = Bundle By Name(cluster=w1543, "MethodNames"=string[] [], "MethodVIs"=w1523, "MethodItemNames"=w1522, "Methods.DynamicDispatch"=w1517) -> (w1542:T18)
                n611 = local write ".vim"(FALSE (".vim")) -> ()
                n612 = Bundle(cluster=w1553, "Left"=w1552, "Top"=w1551, "Right"=w1550) -> (w1549:T23)  [unwired: 1 in]
                n613 = property class="VI"("Front Panel.PanelBounds"=w1549) -> ()  [unwired: 2 in, 2 out]
                n614 = property on="_MethodName" class="Str"("Caption.Text"=w1526) -> ()  [unwired: 2 in, 2 out]
                n615 = property on="_Method" class="LstBox (strict)"("Item Names"=w1522, "Item Symbols"=w1520, "Top Row"=0) -> ()  [unwired: 2 in, 2 out]
              }
              event "PropertyNodeMethodNaming": Value Change {
                n616 = event-data() -> ()  [unwired: 1 in, 4 out]
                n617 = Unbundle By Name(w1631) -> ("PropertyNodeMethods"=w1630:T12[])
                n618 = call <resource>:"BaseProvider_IniFileSettings.vi"() -> ("IniFileSettings"=w1638:T34)  [unwired: 18 in, 1 out]
                n619 = Unbundle By Name(w1638) -> ("UseGetSetForPropertyNodeMethods"=w1637:bool)
                n620 = Equal?(x="PropertyNodeMethodNaming", y=enum16{"Read/Write Naming", "Get/Set Naming"}."Get/Set Naming") -> (x = y?=w1629:bool)
                n621 = call <resource>:"RenamePropertyMethods.vi"("RenameToGet/Set"=w1629, "PropertyNodeMethods"=w1630) -> ("Array"=w1628:T12[])  [unwired: 9 in]
                n622 = for {
                  tunnel: w1628 -> [w1642] mode=indexing
                  tunnel: [w1641] -> w1627 mode=indexing
                  n623 = Unbundle By Name(w1642) -> ("Name"=w1641:string)
                }
                n624 = Not Equal?(x=w1629, y=w1637) -> (x != y?=w1636:bool)
                n625 = local read "_Property"() -> (w1626:string[])
                n626 = Bundle By Name(cluster=w1638, "UseGetSetForPropertyNodeMethods"=w1629) -> (w1639:T34)
                n627 = property on="_Property" class="Tree (strict)"("Val(Sgnl)"=w1626) -> ()  [unwired: 2 in, 2 out]
                n628 = property on="_Method" class="LstBox (strict)"("Item Names"=w1627) -> ()  [unwired: 2 in, 2 out]
                n629 = Bundle By Name(cluster=w1633, "MethodItemNames"=w1627) -> (w1632:T18)
                n630 = case shown="True" w1636 {
                  tunnel: w1639 -> [_ w1644]
                  frame False {
                  }
                  frame True {
                    n631 = call <resource>:"BaseProvider_IniFileSettings.vi"("IniFileSettings"=w1644, "Action"=enum16{"Read", "Load", "Save"}."Save") -> ()  [unwired: 16 in, 2 out]
                  }
                }
              }
              event ".vim": Value Change {
                n632 = event-data() -> ()  [unwired: 1 in, 4 out]
              }
              event "Help": Value Change {
                n633 = event-data() -> ()  [unwired: 1 in, 2 out]
                n634 = call <resource>:"GOOP_HelpMain.vi"() -> ()  [unwired: 12 in]
              }
              event "_ShowContextHelp": Value Change {
                n635 = event-data() -> ("NewVal"=w1651:bool)  [unwired: 1 in]
                n636 = Control Help Window(1:w1651) -> ()  [unwired: 1 in]
              }
            }
            n637 = local read "_Property"() -> (w508:string[])
            n638 = Array Size(array=w508) -> (size(s)=w507:i32)
            n639 = Greater Or Equal?(x=w507, y=2) -> (x >= y?=w506:bool)
            n640 = Select(t=T19."Disabled and Grayed Out" ("Disabled"), s=w506, f=T19."Enabled" ("Disabled")) -> (s? t:f=w503:T19)
            n641 = property on="_MethodIconName" class="Str"("DisabledEnum"=w503) -> ()  [unwired: 2 in, 2 out]
            n642 = Unbundle By Name(w511) -> ("MethodNames"=w510:string[])
            n643 = stacked-sequence {
              tunnel: w515 -> [_]
              tunnel: w511 -> [w525]
              tunnel: w510 -> [w520]
              frame #0 {
                n644 = local read "_MethodType"() -> (w527:T2)
                n645 = Unbundle By Name(w525) -> ("ClassVIs"=w517:string[])
                n646 = local read "_MethodName"() -> (w516:string)
                n647 = local read "_MethodIconName"() -> (w529:string)
                n648 = local read "_Method"() -> (w528:i32[])
                n649 = Empty Array?(array=w520) -> (empty?=w522:bool)
                n650 = case shown="\"Property Method\", \"Property Node\"" w527 {
                  tunnel: [TRUE w546 w557] -> w526
                  frame "Normal Method", Default {
                  }
                  frame "Override Method" {
                    n651 = local read "_OverrideMethods"() -> (w547:i32)
                    n652 = Greater Or Equal To 0?(x=w547) -> (x >= 0?=w546:bool)
                  }
                  frame "Property Method", "Property Node" {
                    n653 = local read "_Property"() -> (w549:string[])
                    n654 = Equal?(x=w549, y="ClassAttribute" ("Left Cell String(Main name)")) -> (x = y?=w554:bool[])
                    n655 = Empty String/Path?(string/path=w549) -> (empty?=w556:bool[])
                    n656 = Equal?(x=w549, y="ObjectAttribute" ("Left Cell String(Main name)")) -> (x = y?=w553:bool[])
                    n657 = Empty Array?(array=w549) -> (empty?=w548:bool)
                    n658 = Build Array (concatenate)(w556, w553, w554, w548) -> (w555:bool[])
                    n659 = Or Array Elements(Boolean array=w555) -> (logical OR=w550:bool)
                    n660 = Not(x=w550) -> (.not. x?=w557:bool)
                  }
                }
                n661 = Build Array(w516) -> (w521:string[])
                n662 = Empty Array?(array=w528) -> (empty?=w523:bool)
                n663 = Select(t=w521, s=w522, f=w520) -> (s? t:f=w519:string[])
                n664 = for {
                  tunnel: w517 -> [w541]
                  tunnel: [w535] -> w518
                  tunnel: w519 -> [w537] mode=indexing
                  stop <- w535 stop-if-true
                  n665 = To Lower Case(string=w541) -> (all lower case string=w539:string[])
                  n666 = Match Pattern(string=w537, regular expression="\\2E[Vv][Ii]") -> (before substring=w543:string)  [unwired: 1 in, 3 out]
                  n667 = Concatenate Strings(w543, ".vi" ("string")) -> (w536:string)
                  n668 = To Lower Case(string=w536) -> (all lower case string=w538:string)
                  n669 = Search 1D Array(1D array=w539, element=w538) -> (index of element=w540:i32)  [unwired: 1 in]
                  n670 = Greater Or Equal To 0?(x=w540) -> (x >= 0?=w535:bool)
                }
                n671 = Empty String/Path?(string/path=w529) -> (empty?=w531:bool)
                n672 = Empty String/Path?(string/path=w516) -> (empty?=w530:bool)
                n673 = Compound Arithmetic op=AND(invert w531, invert w530, invert w523, w526, invert w518) -> (w532:bool)
                n674 = property on="_DubMethodName" class="Str"("Visible"=w518) -> ()  [unwired: 2 in, 2 out]
                n675 = Select(t=u8 0, s=w532, f=u8 2 ("Disabled")) -> (s? t:f=w524:u8)
                n676 = property on="_CreateOpenClass" class="Bool"("Disabled"=w524) -> ()  [unwired: 2 in, 2 out]
                n677 = property on="_CreateMethod" class="Bool"("Disabled"=w524) -> ()  [unwired: 2 in, 2 out]
              }
            }
            n678 = Bundle By Name(cluster=w511, "Cancel"=w513, "Open"=w512, "OverrideMethod"=w501) -> (w514:T18)
          }
          frame "UpdateMethodSettings" {
            n679 = local read "_Visibility"() -> (w1687:T7)
            n680 = case shown="\"Private\"" w1687 {
              tunnel: [TRUE TRUE FALSE FALSE] -> w1682
              tunnel: [w1732 w1734 w1736 w1738] -> w1683
              frame "Public", Default {
                n681 = call <resource>:"GDSControl_Enable.vi"() -> ("Enable Property"=w1732:T19)  [unwired: 11 in]
              }
              frame "Protected" {
                n682 = call <resource>:"GDSControl_Enable.vi"() -> ("Enable Property"=w1734:T19)  [unwired: 11 in]
              }
              frame "Private" {
                n683 = call <resource>:"GDSControl_Disable.vi"() -> ("Enable Property"=w1736:T19)  [unwired: 11 in]
              }
              frame "Community" {
                n684 = call <resource>:"GDSControl_Disable.vi"() -> ("Enable Property"=w1738:T19)  [unwired: 11 in]
              }
            }
            n685 = Unbundle By Name(w1663) -> ("TemplateSettings.MustCallParent"=w1684:enum8{"False", "True", "Mixed"}, "TemplateSettings.MustOverride"=w1685:enum8{"False", "True", "Mixed"}, "TemplateSettings.DynamicDispatch"=w1686:enum8{"False", "True", "Mixed"})
            n686 = Unbundle By Name(w1663) -> ("Methods.DynamicDispatch"=w1660:T14[])
            n687 = local read "_Method"() -> (w1662:i32[])
            n688 = case shown="\"Mixed\"" w1684 {
              tunnel: [TRUE ("Value") FALSE w1716] -> w1670
              tunnel: w1683 -> [_ _ w1717]
              tunnel: [w1712 w1714 w1717] -> w1671
              frame "True" {
                n689 = call <resource>:"GDSControl_Disable.vi"() -> ("Enable Property"=w1712:T19)  [unwired: 11 in]
              }
              frame "False" {
                n690 = call <resource>:"GDSControl_Disable.vi"() -> ("Enable Property"=w1714:T19)  [unwired: 11 in]
              }
              frame "Mixed" {
                n691 = property on="_MustCallParent" class="Bool (strict)"() -> ("Value"=w1716:bool)  [unwired: 2 in, 2 out]
              }
            }
            n692 = case shown="\"Mixed\"" w1685 {
              tunnel: [TRUE ("Value") FALSE w1722] -> w1674
              tunnel: w1683 -> [_ _ w1723]
              tunnel: [w1718 w1720 w1723] -> w1673
              frame "True" {
                n693 = call <resource>:"GDSControl_Disable.vi"() -> ("Enable Property"=w1718:T19)  [unwired: 11 in]
              }
              frame "False" {
                n694 = call <resource>:"GDSControl_Disable.vi"() -> ("Enable Property"=w1720:T19)  [unwired: 11 in]
              }
              frame "Mixed" {
                n695 = property on="_MustOverride" class="Bool (strict)"() -> ("Value"=w1722:bool)  [unwired: 2 in, 2 out]
              }
            }
            n696 = case shown="\"Mixed\"" w1686 {
              tunnel: w1682 -> [w1725 _ w1730]
              tunnel: [w1725 FALSE w1728] -> w1672
              tunnel: w1683 -> [_ _ w1731]
              tunnel: [w1724 w1726 w1731] -> w1659
              frame "True" {
                n697 = call <resource>:"GDSControl_Disable.vi"() -> ("Enable Property"=w1724:T19)  [unwired: 11 in]
              }
              frame "False" {
                n698 = call <resource>:"GDSControl_Disable.vi"() -> ("Enable Property"=w1726:T19)  [unwired: 11 in]
              }
              frame "Mixed" {
                n699 = property on="_DynamicDispatch" class="Bool (strict)"() -> ("Value"=w1729:bool)  [unwired: 2 in, 2 out]
                n700 = And(x=w1730, y=w1729) -> (x .and. y?=w1728:bool)
              }
            }
            n701 = Index Array(array=w1662) -> (element=w1661:i32)  [unwired: 1 in]
            n702 = Index Array(array=w1660, index=w1661) -> (element=w1655:T14)
            n703 = case shown="\"AlwaysOn\"" w1655 {
              tunnel: w1659 -> [w1692 _]
              tunnel: [w1692 w1693] -> w1658
              frame Default {
              }
              frame "AlwaysOn" {
                n704 = call <resource>:"GDSControl_Enable.vi"() -> ("Enable Property"=w1693:T19)  [unwired: 11 in]
              }
            }
            n705 = local read "_MethodType"() -> (w1675:T2)
            n706 = case shown="\"Override Method\"" w1675 {
              tunnel: w1671 -> [w1699 _]
              tunnel: [w1699 w1702] -> w1669
              tunnel: w1670 -> [w1698 _]
              tunnel: [w1698 TRUE ("Value")] -> w1668
              tunnel: w1673 -> [w1696 _]
              tunnel: [w1696 w1702] -> w1667
              tunnel: w1674 -> [w1697 w1701]
              tunnel: [w1697 w1701] -> w1666
              tunnel: w1658 -> [w1695 _]
              tunnel: [w1695 w1702] -> w1665
              tunnel: w1672 -> [w1694 w1700]
              tunnel: [w1694 w1700] -> w1664
              frame Default {
              }
              frame "Override Method" {
                n707 = call <resource>:"GDSControl_Disable.vi"() -> ("Enable Property"=w1702:T19)  [unwired: 11 in]
              }
            }
            n708 = local read ".vim"() -> (w1681:bool)
            n709 = case shown="False" w1681 {
              tunnel: w1669 -> [w1709 _]
              tunnel: [w1709 w1710] -> w1680
              tunnel: w1668 -> [w1708 _]
              tunnel: [w1708 w1711] -> w1679
              tunnel: w1667 -> [w1706 _]
              tunnel: [w1706 w1710] -> w1677
              tunnel: w1666 -> [w1707 _]
              tunnel: [w1707 w1711] -> w1676
              tunnel: w1665 -> [w1705 _]
              tunnel: [w1705 w1710] -> w1657
              tunnel: w1664 -> [w1704 _]
              tunnel: [w1704 w1711] -> w1678
              frame False {
              }
              frame True {
                w1711 = FALSE ("Value")
                n710 = call <resource>:"GDSControl_Disable.vi"() -> ("Enable Property"=w1710:T19)  [unwired: 11 in]
              }
            }
            n711 = case shown="\"AlwaysOff\"" w1655 {
              tunnel: w1657 -> [w1690 _]
              tunnel: [w1690 w1691] -> w1656
              frame Default {
              }
              frame "AlwaysOff" {
                n712 = call <resource>:"GDSControl_Disable.vi"() -> ("Enable Property"=w1691:T19)  [unwired: 11 in]
              }
            }
            n713 = property on="_MustOverride" class="Bool (strict)"("DisabledEnum"=w1677, "Value"=w1676) -> ()  [unwired: 2 in, 2 out]
            n714 = property on="_DynamicDispatch" class="Bool (strict)"("Disabled"=w1656, "Value"=w1678) -> ()  [unwired: 2 in, 2 out]
            n715 = property on="_MustCallParent" class="Bool (strict)"("Disabled"=w1680, "Value"=w1679) -> ()  [unwired: 2 in, 2 out]
          }
          frame "UpdateMethodTemplateImage" {
            n716 = Unbundle By Name(w1741) -> ("MethodItemNames"=w1763:string[])
            n717 = local read "_Method"() -> (w1746:i32[])
            n718 = Unbundle By Name(w1741) -> ("MethodVIs"=w1750:path[])
            n719 = Index Array(array=w1746) -> (element=w1749:i32)  [unwired: 1 in]
            n720 = property on="MethodTemplateImage" class="Pict"() -> ("Draw Area Size"=w1745:T44)  [unwired: 2 in, 2 out]
            n721 = Index Array(array=w1763, index=w1749) -> (element=w1762:string)
            n722 = Index Array(array=w1750, index=w1749) -> (element=w1748:path)
            n723 = call <resource>:"GetMethodImage.vi"("MethodVI"=w1748, "MethodName"=w1762) -> ("MethodImage"=w1742:T16)  [unwired: 8 in, 1 out]
            n724 = Unbundle By Name(w1745) -> ("Width"=w1761:u32, "Height"=w1760:u32)
            n725 = To Word Integer(number=w1761) -> (16bit integer=w1754:i16)
            n726 = Unbundle By Name(w1742) -> ("Rectangle.right"=w1753:i16, "Rectangle.bottom"=w1751:i16)
            n727 = To Word Integer(number=w1760) -> (16bit integer=w1752:i16)
            n728 = Unbundle By Name(w1742) -> ("Rectangle"=w1759:T45)
            n729 = Subtract(x=w1754, y=w1753) -> (x-y=w1756:i16)
            n730 = Subtract(x=w1752, y=w1751) -> (x-y=w1757:i16)
            n731 = Max & Min(x=w1756, y=w1757) -> (min(x,y)=w1755:i16)  [unwired: 1 out]
            n732 = case shown="..-1" w1755 {
              tunnel: w1759 -> [_ w1781]
              tunnel: w1742 -> [w1773 w1779]
              tunnel: [w1773 w1777] -> w1758
              tunnel: w1757 -> [_ w1776]
              tunnel: w1756 -> [_ w1775]
              tunnel: [w1766 1.0] -> w1744
              tunnel: w1754 -> [w1772 _]
              tunnel: w1753 -> [w1771 _]
              tunnel: w1752 -> [w1770 _]
              tunnel: w1751 -> [w1769 _]
              tunnel: [T31 {"Horizontal"=0, "Vertical"=0} ("Origin") _] -> w1743
              frame ..-1 {
                n733 = Divide(x=w1772, y=w1771) -> (x/y=w1768:dbl)
                n734 = Divide(x=w1770, y=w1769) -> (x/y=w1767:dbl)
                n735 = Max & Min(x=w1768, y=w1767) -> (min(x,y)=w1766:dbl)  [unwired: 1 out]
              }
              frame Default {
                n736 = expression code="x/2"(w1775) -> (w1783:i16)
                n737 = expression code="y/2"(w1776) -> (w1782:i16)
                n738 = Bundle(w1783, w1782, w1783, w1782) -> (w1780:cluster{i16, i16, i16, i16})  [unwired: 1 in]
                n739 = Add(x=w1781, y=w1780) -> (x+y=w1778:cluster{i16, i16, i16, i16})
                n740 = Bundle By Name(cluster=w1779, "Rectangle"=w1778) -> (w1777:T16)
              }
            }
            n741 = call <vilib>:"Draw Flattened Pixmap.vi"("image data"=w1758) -> ("new picture"=w1740:picture)  [unwired: 8 in]
            n742 = property on="MethodTemplateImage" class="Pict"("ZoomFactor"=w1744, "Origin"=w1743, "Value"=w1740) -> ()  [unwired: 2 in, 2 out]
          }
          frame "PlaceIcon" {
            n743 = Unbundle By Name(w1787) -> ("Icons"=w1789:T16[], "IconSelected"=w1790:i32)
            n744 = Index Array(array=w1789, index=w1790) -> (element=w1791:T16)
            n745 = call <resource>:"GDSIconEditor_ImageDataTo8Bit.vi"("image data"=w1791) -> ("8-bit pixmap"=w1784:u8[][])  [unwired: 7 in, 3 out]
            n746 = Bundle By Name(cluster=w1787, "BgIcon"=w1784, "BgIconOffset"=cluster{"X":i32, "Y":i32} {"X"=0, "Y"=0}) -> (w1788:T18)
          }
          frame "CreateMethodIcons" {
            w1821 = T29 {"BgIcon"=[], "BgIconOffset"={"X"=0, "Y"=0}, "BgIconMask"=[], "ColorsOkayforiconToBeOnTopOf"=[]}  # BgIcon
            n747 = Unbundle By Name(w1798) -> ("Frame thickness"=w1819:i32, "ConnectorPaneHeight"=w1811:i32[], "BodyIconHeight"=w1812:i32)
            n748 = Unbundle By Name(w1798) -> ("Frame"=w1803:u32, "Frame thickness"=w1804:i32, "HeaderIcon"=w1815:u8[][])
            n749 = local read "_IconSize"() -> (w1816:u16)
            n750 = local read "_BodyBk"() -> (w1809:T1)
            n751 = Unbundle By Name(w1809) -> ("Color"=w1828:u32)
            n752 = Unbundle By Name(w1798) -> ("BgIcon"=w1822:u8[][], "BgIconOffset"=w1823:cluster{"X":i32, "Y":i32}, "BgIconMask"=w1825:u8[], "HeaderBkColor"=w1826:u32)
            n753 = Unbundle By Name(w1798) -> ("MethodNames"=w1831:string[])
            n754 = Unbundle By Name(w1798) -> ("BodyIconHeight"=w1838:i32, "BodyIconWidth"=w1837:i32)
            n755 = case shown="1" w1816 {
              tunnel: w1815 -> [w1852 _]
              tunnel: [w1852 _] -> w1805
              frame Default {
              }
              frame 1 {
              }
            }
            n756 = call <resource>:"GDSLvIcon_Convert24bitTo8bitColor.vi"("Color 24bit In"=w1826) -> ("Color out(256)"=w1827:u8)  [unwired: 15 in, 3 out]
            n757 = call <resource>:"GDSLvIcon_Convert24bitTo8bitColor.vi"("Color 24bit In"=w1828) -> ("Color out(256)"=w1829:u8)  [unwired: 15 in, 3 out]
            n758 = Not Equal?(x=u16 0, y=w1816) -> (x != y?=w1817:bool)
            n759 = Array Size(array=w1805) -> (size(s)=w1813:i32[])
            n760 = Build Array(w1827, w1829) -> (w1824:u8[])
            n761 = Index Array(array=w1813) -> (element=w1814:i32)  [unwired: 1 in]
            n762 = Select(t=0, s=w1817, f=0) -> (s? t:f=w1801:i32)
            n763 = Multiply(x=w1819, y=u32 2) -> (x*y=w1820:u32)
            n764 = case shown="Default" w1816 {
              selector: w1816 -> [_ w1840 _]
              tunnel: w1812 -> [_ _ _]
              tunnel: w1811 -> [_ w1847 w1850]
              tunnel: [32 ("ImageRows(32)") w1844 w1851] -> w1802
              tunnel: w1814 -> [_ w1843 _]
              tunnel: w1820 -> [_ w1842 w1848]
              frame 0 {
              }
              frame Default {
                n765 = Decrement(x=w1840) -> ()  [unwired: 1 out]
                n766 = Array Subset(array=w1847, length=w1840) -> (w1846:i32[])  [unwired: 1 in]
                n767 = Add Array Elements(numeric array=w1846) -> (sum=w1845:i32)
                n768 = Increment(x=w1842) -> (x+1=w1841:u32)
                n769 = Compound Arithmetic op=ADD(w1841, w1843, w1845) -> (w1844:u32)
              }
              frame 1 {
                n770 = Index Array(array=w1850) -> (element=w1849:i32)  [unwired: 1 in]
                n771 = Compound Arithmetic op=ADD(w1848, w1849) -> (w1851:u32)
              }
            }
            n772 = Bundle By Name(cluster=w1821, "BgIcon"=w1822, "BgIconOffset"=w1823, "BgIconMask"=w1825, "ColorsOkayforiconToBeOnTopOf"=w1824) -> (w1806:T29)
            n773 = local read "_MethodIconName"() -> (w1800:string)
            n774 = local read "_Property"() -> (w1795:string[])
            n775 = Array Size(array=w1795) -> (size(s)=w1794:i32)
            n776 = Greater Or Equal?(x=w1794, y=2) -> (x >= y?=w1793:bool)
            n777 = Unbundle By Name(w1798) -> ("Offset"=w1799:cluster{"X":i32, "Y":i32})
            n778 = for {
              tunnel: w1838 -> [w1881]
              tunnel: w1837 -> [w1880]
              shift-right: [w1870] -> w1834
              shift-left: w1835 -> [w1875]
              shift-right: [w1873] -> w1830
              shift-left: u8[][] [] -> [w1874]
              tunnel: w1831 -> [w1856] mode=indexing
              tunnel: w1806 -> [w1869]
              tunnel: w1805 -> [w1868]
              tunnel: w1804 -> [w1867]
              tunnel: w1803 -> [w1866]
              tunnel: w1802 -> [w1865]
              tunnel: w1801 -> [w1864]
              tunnel: w1800 -> [w1860]
              tunnel: w1799 -> [w1862]
              tunnel: "^Read|^Get|^Write|^Set|" ("regular expression") -> [w1859]
              tunnel: w1793 -> [w1853]
              n779 = xnode "Match Regular Expression"("input string"=w1856, "regular expression"=w1859) -> ("whole match"=w1861:string)  [unwired: 4 in, 4 out]
              n780 = xnode "Match Regular Expression"("input string"=w1860, "regular expression"=w1859) -> ("before match"=w1858:string, "after match"=w1857:string)  [unwired: 4 in, 3 out]
              n781 = Concatenate Strings(w1861, w1858, w1857) -> (w1855:string)
              n782 = Select(t=w1856, s=w1853, f=w1855) -> (s? t:f=w1854:string)
              n783 = local read "_BodyBk"() -> (w1879:T1)
              n784 = local read "_BodyText"() -> (w1877:T1)
              n785 = local read "_FontCompression"() -> (w1884:enum16{"Auto", "On", "Off"})
              n786 = local read "_CapitalOnly"() -> (w1883:bool)
              n787 = Bundle By Name(cluster=T26 {"Text"="", "Allow Only Capital Chars"=FALSE, "Compression"=enum."Auto", "Alignment"=enum."Center"} ("Text"), "Text"=w1854, "Allow Only Capital Chars"=w1883, "Compression"=w1884) -> (w1882:T26)
              n788 = Unbundle(w1877) -> ("Color"=w1876:u32)  [unwired: 1 out]
              n789 = Unbundle(w1879) -> ("Color"=w1878:u32)  [unwired: 1 out]
              n790 = call <resource>:"GDSLvIcon_GenerateIconText.vi"("Text"=w1882, "TextPixelHeight(5-30)"=w1881, "Foreground color"=w1876, "Background color"=w1878, "error in (no error)"=w1875, "Offset"=w1862, "Text Pixel width(32-FrameThicknes*2))"=w1880) -> ("TextOut"=w1872:u8[][], "error out"=w1871:errorcluster)  [unwired: 8 in, 3 out]
              n791 = call <resource>:"GDSLvIcon_CreateIconPicture.vi"("FrameColor"=w1866, "FrameThickness(1)"=w1867, "HeaderIconIn"=w1868, "BodyIconIn"=w1872, "error in (no error)"=w1871, "ImageRows(32)"=w1865, "RowStart(0)"=w1864, "BgIcon"=w1869) -> ("BodyIconOut"=w1863:u8[][], "error out"=w1870:errorcluster)  [unwired: 6 in, 4 out]
              n792 = Build Array (concatenate)(w1874, w1863) -> (w1873:u8[][])
            }
            n793 = Bundle By Name(cluster=w1798, "BodyIconOut"=w1830) -> (w1836:T18)
          }
          frame "UpdateOverRideMethods" {
            w2108 = TRUE ("Visible")
            n794 = Unbundle By Name(w2111) -> ("OverRideLookUpDone"=w2114:bool)
            n795 = local write "_OverrideMethods"(-1 ("Override Methods")) -> ()
            n796 = property on="_Property" class="Tree (strict)"("Visible"=FALSE) -> ()  [unwired: 2 in, 2 out]
            n797 = property on="_OverrideMethods" class="LstBox (strict)"("Visible"=w2108) -> ()  [unwired: 2 in, 2 out]
            n798 = property on="Filter" class="Str"("Visible"=w2108) -> ()  [unwired: 2 in, 2 out]
            n799 = case shown="False" w2114 {
              tunnel: w2116 -> [w2131 w2148]
              tunnel: w2115 -> [w2140 _]
              tunnel: [w2128 w2148] -> w2109
              tunnel: w2111 -> [w2134 w2147]
              tunnel: [w2133 w2147] -> w2110
              tunnel: [w2127 _] -> _
              frame False {
                w2125 = "" ("Method Name")
                n800 = call <vilib>:"Set Busy.vi"("error in (no error)"=w2131) -> ("error out"=w2130:errorcluster)  [unwired: 9 in, 1 out]
                n801 = property on="_Loading" class="Str"(error in=w2130, "Visible"=TRUE) -> (error out=w2138:errorcluster)  [unwired: 1 in, 1 out]
                n802 = call <resource>:"GOOP_GetOverrideMethods.vi"("LvClassItem"=w2140, "error in (no error)"=w2138) -> ("IsMustOverrideVI"=w2118:bool[], "IsAPropertyDefinitionVI"=w2124:bool[], "DynamicMethods(Names)"=w2120:string[], "DynamicMehods(Paths)"=w2132:path[], "Scope"=w2129:T33, "ConnectorPaneHeight"=w2126:i32[], "error out"=w2136:errorcluster)  [unwired: 11 in]
                n803 = for {
                  tunnel: w2120 -> [w2145] mode=indexing
                  tunnel: [w2144] -> w2119 mode=indexing
                  tunnel: w2118 -> [w2143] mode=indexing
                  n804 = Append True/False String(1:w2143, 2:"", 3:"*", 4:w2145) -> (0:w2144:string)
                }
                n805 = local write "_MethodName"(w2125) -> ()
                n806 = local write "_MethodIconName"(w2125) -> ()
                n807 = local write "Filter"("" ("Filter")) -> ()
                n808 = property on="_OverrideMethods" class="LstBox (strict)"("Item Names"=w2119, "Top Row"=0) -> ()  [unwired: 2 in, 2 out]
                n809 = for {
                  tunnel: w2120 -> [_] mode=indexing
                  tunnel: [w2146] -> w2121 mode=indexing
                  i -> [w2146]
                }
                n810 = Bundle By Name(cluster=w2134, "OverrideMethodsIdx"=w2121, "OverrideMethodsNames"=w2120, "OverRideLookUpDone"=TRUE, "AllOverrideMethods"=w2132, "OverrideScope"=w2129, "ConnectorPaneHeight"=w2126, "IsAPropertyDefinitionVI"=w2124) -> (w2133:T18)
                n811 = property on="_Loading" class="Str"(error in=w2136, "Visible"=FALSE) -> (error out=w2128:errorcluster)  [unwired: 1 in, 1 out]
                n812 = call <vilib>:"Unset Busy.vi"("error in (no error)"=w2128) -> ("error out"=w2127:errorcluster)  [unwired: 10 in]
              }
              frame True {
              }
            }
          }
          frame "UpdateProperties" {
            (unwired) "" ("Property")
            w2149 = FALSE ("Visible")
            n813 = Unbundle By Name(w2156) -> ("PropertyLookUpDone"=w2157:bool)
            n814 = case shown="False" w2157 {
              tunnel: w2159 -> [w2167 w2173]
              tunnel: w2158 -> [w2172 _]
              tunnel: [w2162 w2173] -> w2150
              tunnel: w2152 -> [w2163 _]
              tunnel: [w2161 _] -> _
              frame False {
                w2168 = "" ("Method Name")
                n815 = control-ref of="_Property"() -> (w2165:refnum<vi>)
                n816 = call <vilib>:"Set Busy.vi"("error in (no error)"=w2167) -> ("error out"=w2166:errorcluster)  [unwired: 9 in, 1 out]
                n817 = property on="_Loading" class="Str"(error in=w2166, "Visible"=TRUE) -> (error out=w2170:errorcluster)  [unwired: 1 in, 1 out]
                n818 = call-dynamic "GetClassProperties.vi"("reference in"=w2163, "LvClassItem"=w2172, "TreeControl"=w2165, "error in (no error)"=w2170) -> ("error out"=w2164:errorcluster)  [unwired: 14 in, 1 out]
                n819 = local write "_MethodName"(w2168) -> ()
                n820 = local write "_MethodIconName"(w2168) -> ()
                n821 = property on="_Loading" class="Str"(error in=w2164, "Visible"=FALSE) -> (error out=w2162:errorcluster)  [unwired: 1 in, 1 out]
                n822 = call <vilib>:"Unset Busy.vi"("error in (no error)"=w2162) -> ("error out"=w2161:errorcluster)  [unwired: 10 in]
              }
              frame True {
              }
            }
            n823 = property on="_Property" class="Tree (strict)"("Visible"=TRUE) -> ()  [unwired: 2 in, 2 out]
            n824 = property on="_OverrideMethods" class="LstBox (strict)"("Visible"=w2149) -> ()  [unwired: 2 in, 2 out]
            n825 = property on="Filter" class="Str"("Visible"=w2149) -> ()  [unwired: 2 in, 2 out]
            n826 = local write "_Property"(string[] [] ("_Property")) -> ()
            n827 = Bundle By Name(cluster=w2156, "PropertyLookUpDone"=TRUE ("OverRideLookUpDone")) -> (w2155:T18)
          }
          frame "UpdateCurrentIconBgColors" {
            w2175 = T29 {"BgIcon"=[], "BgIconOffset"={"X"=0, "Y"=0}, "BgIconMask"=[], "ColorsOkayforiconToBeOnTopOf"=[]}  # BgIcon
            n828 = local read "_BodyBk"() -> (w2180:T1)
            n829 = Unbundle By Name(w2180) -> ("Color"=w2178:u32)
            n830 = call <resource>:"GDSLvIcon_Convert24bitTo8bitColor.vi"("Color 24bit In"=w2178) -> ("Color out(256)"=w2179:u8)  [unwired: 15 in, 3 out]
            n831 = Unbundle By Name(w2177) -> ("BgIcon"=w2181:u8[][], "BgIconOffset"=w2182:cluster{"X":i32, "Y":i32}, "BgIconMask"=w2184:u8[], "HeaderBkColor"=w2185:u32)
            n832 = call <resource>:"GDSLvIcon_Convert24bitTo8bitColor.vi"("Color 24bit In"=w2185) -> ("Color out(256)"=w2186:u8)  [unwired: 15 in, 3 out]
            n833 = Build Array(w2186, w2179) -> (w2183:u8[])
            n834 = Bundle By Name(cluster=w2175, "BgIcon"=w2181, "BgIconOffset"=w2182, "BgIconMask"=w2184, "ColorsOkayforiconToBeOnTopOf"=w2183) -> (w2187:T29)
            n835 = Bundle By Name(cluster=w2177, "CurrentIcon"=w2187) -> (w2176:T18)
          }
          frame "Generate icon", "UpdateIcon" {
            (unwired) T20."1 c-term high"  # _IconSize
            n836 = local read "_IconSize"() -> (w2228:u16)
            n837 = local read "_MethodIconName"() -> (w2201:string)
            n838 = local read "_MethodType"() -> (w2202:T2)
            n839 = Unbundle By Name(w2196) -> ("Offset"=w2214:cluster{"X":i32, "Y":i32}, "Frame"=w2230:u32, "Frame thickness"=w2243:i32, "HeaderIcon"=w2233:u8[][])
            n840 = Unbundle By Name(w2196) -> ("ConnectorPaneHeight"=w2229:i32[], "BodyIconHeight"=w2227:i32, "BodyIconWidth"=w2238:i32, "Splitter0px"=w2189:bool)
            n841 = Unbundle By Name(w2196) -> ("CurrentIcon"=w2206:T29)
            n842 = Unbundle By Name(w2196) -> ("HeaderBkColor"=w2193:u32)
            n843 = case shown="\"Property Node\"" w2202 {
              tunnel: w2201 -> [w2250 w2253]
              tunnel: [w2250 w2251] -> w2200
              frame Default {
              }
              frame "Property Node" {
                n844 = Match Pattern(string=w2253, regular expression="/") -> (before substring=w2251:string)  [unwired: 1 in, 3 out]
              }
            }
            n845 = case shown="Default" w2228 {
              tunnel: w2233 -> [w2295 _]
              tunnel: [w2295 _] -> w2224
              frame Default {
              }
              frame 1 {
              }
            }
            n846 = Array Size(array=w2224) -> (size(s)=w2225:i32[])
            n847 = Index Array(array=w2225) -> (element=w2223:i32)  [unwired: 1 in]
            n848 = Multiply(x=w2230, y=u32 2) -> (x*y=w2205:u32)
            n849 = Increment(x=w2205) -> (x+1=w2226:u32)
            n850 = case shown="Default" w2228 {
              selector: w2228 -> [_ w2263 _]
              tunnel: w2227 -> [w2257 _ _]
              tunnel: [w2257 w2262 w2283] -> w2222
              tunnel: w2229 -> [_ w2264 w2284]
              tunnel: [32 ("ImageRows(32)") w2260 w2285] -> w2199
              tunnel: w2223 -> [_ w2259 _]
              tunnel: w2226 -> [_ w2261 w2286]
              tunnel: w2205 -> [_ w2258 w2282]
              frame 0 {
              }
              frame Default {
                n851 = disable-structure shown="Enabled" {
                  disable-tunnel: w2264 -> [w2272 w2276]
                  disable-tunnel: w2263 -> [w2271 w2273]
                  disable-tunnel: [w2269 w2277] -> w2262
                  disable-tunnel: w2261 -> [w2268 _]
                  disable-tunnel: [w2267 w2278] -> w2260
                  disable-tunnel: w2259 -> [w2265 w2274]
                  disable-tunnel: w2258 -> [_ w2275]
                  frame Disabled {
                    n852 = Decrement(x=w2271) -> (x-1=w2266:u16)
                    n853 = Array Subset(array=w2272, length=w2266) -> (w2270:i32[])  [unwired: 1 in]
                    n854 = Add Array Elements(numeric array=w2270) -> (sum=w2269:i32)
                    n855 = Compound Arithmetic op=ADD(w2268, w2265, w2269) -> (w2267:u32)
                  }
                  frame Enabled {
                    n856 = Array Subset(array=w2276, length=w2273) -> (w2279:i32[])  [unwired: 1 in]
                    n857 = Add Array Elements(numeric array=w2279) -> (sum=w2278:i32)
                    n858 = Increment(x=w2275) -> (x+1=w2280:u32)
                    n859 = Compound Arithmetic op=ADD(w2280, w2274) -> (w2281:u32)
                    n860 = Subtract(x=w2278, y=w2281) -> (x-y=w2277:u32)
                  }
                }
              }
              frame 1 {
                n861 = disable-structure shown="Enabled" {
                  disable-tunnel: w2286 -> [w2290 _]
                  disable-tunnel: [w2289 w2292] -> w2285
                  disable-tunnel: w2284 -> [w2288 w2294]
                  disable-tunnel: [w2287 w2291] -> w2283
                  disable-tunnel: w2282 -> [_ w2293]
                  frame Disabled {
                    n862 = Index Array(array=w2288) -> (element=w2287:i32)  [unwired: 1 in]
                    n863 = Compound Arithmetic op=ADD(w2290, w2287) -> (w2289:u32)
                  }
                  frame Enabled {
                    n864 = Index Array(array=w2294) -> (element=w2292:i32)  [unwired: 1 in]
                    n865 = Subtract(x=w2292, y=w2293) -> (x-y=w2291:u32)
                  }
                }
              }
            }
            n866 = call <resource>:"GDSLvIcon_Convert24bitTo8bitColor.vi"("Color 24bit In"=w2193) -> ("Color out(256)"=w2194:u8)  [unwired: 15 in, 3 out]
            n867 = local read "_CapitalOnly"() -> (w2246:bool)
            n868 = local read "_BodyText"() -> (w2235:T1)
            n869 = local read "_BodyBk"() -> (w2236:T1)
            n870 = local read "_TextAlignment"() -> (w2221:u16)
            n871 = local read "_FontCompression"() -> (w2247:enum16{"Auto", "On", "Off"})
            n872 = Bundle By Name(cluster=T26 {"Text"="", "Allow Only Capital Chars"=FALSE, "Compression"=enum."Auto", "Alignment"=enum."Center"} ("Text"), "Alignment"=w2221, "Text"=w2200, "Allow Only Capital Chars"=w2246, "Compression"=w2247) -> (w2245:T26)
            n873 = Unbundle(w2235) -> ("Color"=w2234:u32)  [unwired: 1 out]
            n874 = Unbundle(w2236) -> ("Color"=w2191:u32)  [unwired: 1 out]
            n875 = call <resource>:"GDSLvIcon_Convert24bitTo8bitColor.vi"("Color 24bit In"=w2191) -> ("Color out(256)"=w2195:u8)  [unwired: 15 in, 3 out]
            n876 = Build Array(w2194, w2195) -> (w2192:u8[])
            n877 = Unbundle By Name(w2196) -> ("AF"=w2203:bool, "OldOffset.X"=w2216:i32, "OldOffset.Y"=w2215:i32)
            n878 = Bundle By Name(cluster=w2206, "ColorsOkayforiconToBeOnTopOf"=w2192) -> (w2197:T29)
            n879 = Unbundle By Name(w2214) -> ("X"=w2213:i32, "Y"=w2212:i32)
            n880 = call <resource>:"GDSLvIcon_GenerateIconText.vi"("Text"=w2245, "TextPixelHeight(5-30)"=w2222, "Foreground color"=w2234, "Background color"=w2191, "error in (no error)"=w2239, "Offset"=w2214, "Text Pixel width(32-FrameThicknes*2))"=w2238) -> ("X-Limited"=w2218:bool, "Y-Limited"=w2217:bool, "TextOut"=w2237:u8[][], "TextBounds"=w2208:T42, "error out"=w2249:errorcluster)  [unwired: 8 in]
            n881 = call <resource>:"GDSLvIcon_CreateIconPicture.vi"("FrameColor"=w2230, "FrameThickness(1)"=w2243, "HeaderIconIn"=w2224, "BodyIconIn"=w2237, "error in (no error)"=w2249, "ImageRows(32)"=w2199, "BigSizeIcon(x6)"=4, "BgIcon"=w2197, "0px Splitter(False)"=w2189) -> ("BodyIconOut"=w2204:u8[][], "LargeIconPictureOut(x6)"=→"_IconPreview":picture, "BodyOffset"=w2190:cluster{"X":i32, "Y":i32}, "error out"=w2240:errorcluster)  [unwired: 5 in, 2 out]
            n882 = Select(t=w2216, s=w2218, f=w2213) -> (s? t:f=w2219:i32)
            n883 = Select(t=w2215, s=w2217, f=w2212) -> (s? t:f=w2220:i32)
            n884 = Unbundle(w2190) -> ("X"=w2209:i32, "Y"=w2210:i32)
            n885 = case shown="False" w2203 {
              tunnel: ["Idle" "ActorTemplates"] -> w2244
              frame False {
              }
              frame True {
              }
            }
            n886 = Bundle("Y"=w2210, "X"=w2209, "Y"=w2210, "X"=w2209) -> (w2211:cluster{"Y":i32, "X":i32, "Y":i32, "X":i32})  [unwired: 1 in]
            n887 = Add(x=w2211, y=w2208) -> (x+y=w2207:cluster{i32, i32, i32, i32})
            n888 = Bundle By Name(cluster=w2196, "Offset.X"=w2219, "Offset.Y"=w2220, "MethodIcon"=w2237, "IconDetails.IconSize"=w2228, "IconDetails.ImageRows(32)"=w2199, "IconDetails.ConnectorPaneHeight"=w2229, "TextBounds"=w2207, "BodyIconOut"=w2204, "RowStart(0)"=0, "ImageRows(32)"=w2199) -> (w2232:T18)
          }
          frame "ActorTemplates" {
            w2316 = TRUE
            n889 = feedback-in #1(w2316) -> ()
            n890 = feedback #1() -> (w2317:bool)
            n891 = Not Equal?(x=w2316, y=w2317) -> (x != y?=w2315:bool)
            n892 = case shown="True" w2315 {
              tunnel: w2314 -> [_ w2383]
              tunnel: w2300 -> [w2366 w2374]
              tunnel: [w2366 w2371] -> w2304
              frame False {
              }
              frame True {
                n893 = call <resource>:"AF_GetClassAfInfo.vi"("DeriveFromClassRef"=w2383) -> ("AF Folder Path"=w2382:path)  [unwired: 5 in, 5 out]
                n894 = Build Path(base path=w2382, name or relative path="MethodTemplates") -> (appended path=w2369:path)
                n895 = Build Path(base path=w2369, name or relative path="Templates.ini") -> (appended path=w2379:path)
                n896 = call <vilib>:"Open Config Data.vi"("configuration file path"=w2379) -> ("error out"=w2378:errorcluster, "refnum"=w2377:T46)  [unwired: 8 in, 1 out]
                n897 = call <vilib>:"Get Section Names.vi"("error in (no error)"=w2378, "refnum"=w2377) -> ("error out"=w2375:errorcluster, "section names"=w2373:string[], "refnum out"=w2376:T46)  [unwired: 7 in]
                n898 = for {
                  tunnel: w2373 -> [w2389] mode=indexing
                  shift-right: [w2391] -> w2367
                  shift-left: w2375 -> [w2395]
                  shift-right: [w2392] -> w2368
                  shift-left: w2376 -> [w2396]
                  tunnel: [w2385] -> w2372 mode=indexing
                  tunnel: w2369 -> [w2384]
                  n899 = call <vilib>:"Get Key Names.vi"("section"=w2389, "error in (no error)"=w2395, "refnum"=w2396) -> ("error out"=w2393:errorcluster, "key names"=w2390:string[], "refnum out"=w2394:T46)  [unwired: 5 in, 1 out]
                  n900 = for {
                    shift-right: [w2407] -> w2392
                    shift-left: w2394 -> [w2409]
                    shift-right: [w2406] -> w2391
                    shift-left: w2393 -> [w2408]
                    tunnel: w2390 -> [w2397] mode=indexing
                    tunnel: w2389 -> [w2400]
                    tunnel: MethodType."AF-Method" ("Type") -> [w2404]
                    tunnel: T12 {"Type"=enum."Normal", "Name"="", "Path"=path "", "ExtraName"="", "Data"=variant, "DynamicDispatch"=enum."Default"} ("cluster") -> [w2403]
                    tunnel: [w2402] -> w2386 mode=indexing
                    tunnel: w2384 -> [w2401]
                    n901 = Build Path(base path=w2401, name or relative path=w2397) -> (appended path=w2399:path)
                    n902 = call-poly <vilib>:"Read Key.vi"("read raw string? (F)"=TRUE, "section"=w2400, "error in (no error)"=w2408, "key"=w2397, "refnum"=w2409) -> ("error out"=w2406:errorcluster, "value"=w2398:string, "refnum out"=w2407:T46)  [unwired: 3 in, 1 out]
                    n903 = Bundle By Name(cluster=w2403, "Type"=w2404, "Name"=w2398, "Path"=w2399) -> (w2402:T12)
                  }
                  n904 = Bundle(w2386) -> (w2385:cluster{T12[]})  [unwired: 1 in]
                }
                n905 = To Lower Case(string=w2373) -> (all lower case string=w2370:string[])
                n906 = Bundle By Name(cluster=w2374, "AF-MethodNames"=w2370, "AF-Methods"=w2372) -> (w2371:T18)
                n907 = call <vilib>:"Close Config Data.vi"("error in (no error)"=w2367, "refnum"=w2368) -> ()  [unwired: 8 in, 2 out]
              }
            }
            n908 = Unbundle By Name(w2300) -> ("AF"=w2299:bool)
            n909 = local read "_MethodName"() -> (w2318:string)
            n910 = call <vilib>:"Trim Whitespace.vi"("string"=w2318) -> ("trimmed string"=w2312:string)  [unwired: 1 in]
            n911 = To Lower Case(string=w2312) -> (all lower case string=w2311:string)
            n912 = Unbundle By Name(w2304) -> ("AF-MethodNames"=w2313:string[], "AF-Methods"=w2308:cluster{T12[]}[])
            n913 = Search 1D Array(1D array=w2313, element=w2311) -> (index of element=w2301:i32)  [unwired: 1 in]
            n914 = Index Array(array=w2308, index=w2301) -> (element=w2307:cluster{T12[]})
            n915 = Unbundle(w2307) -> (w2306:T12[])
            n916 = Greater Or Equal To 0?(x=w2301) -> (x >= 0?=w2302:bool)
            n917 = feedback-in #2(w2302) -> ()
            n918 = feedback #2() -> (w2310:bool)
            n919 = Compound Arithmetic op=AND(invert w2302, w2310) -> (w2309:bool)
            n920 = case shown="True" w2302 {
              tunnel: w2309 -> [w2325 _]
              tunnel: w2300 -> [w2324 _]
              tunnel: w2306 -> [_ w2357]
              tunnel: w2299 -> [w2323 _]
              tunnel: [w2322 w2355] -> w2298
              tunnel: [w2321 w2354] -> w2297
              tunnel: [w2320 w2353] -> w2296
              frame False {
                n921 = case shown="True" w2325 {
                  tunnel: w2324 -> [w2329 w2336]
                  tunnel: w2323 -> [_ w2333]
                  tunnel: [w2328 w2332] -> w2322
                  tunnel: [w2327 w2331] -> w2321
                  tunnel: [w2326 w2330] -> w2320
                  frame False {
                    n922 = Unbundle By Name(w2329) -> ("MethodItemNames"=w2327:string[], "MethodVIs"=w2328:path[], "Methods.DynamicDispatch"=w2326:T14[])
                  }
                  frame True {
                    n923 = local write "_AddMessageClass"(w2333) -> ()
                    n924 = local read "_MethodType"() -> (w2337:T2)
                    n925 = case shown="\"Normal Method\", Default" w2337 {
                      tunnel: w2336 -> [w2346 w2348 w2350 w2352]
                      tunnel: [w2345 w2347 w2349 w2351] -> w2334
                      frame "Normal Method", Default {
                        n926 = Unbundle By Name(w2346) -> ("NormalMethods"=w2345:T12[])
                      }
                      frame "Override Method" {
                        n927 = Unbundle By Name(w2348) -> ("OverrideMethods"=w2347:T12[])
                      }
                      frame "Property Method" {
                        n928 = Unbundle By Name(w2350) -> ("PropertyMethods"=w2349:T12[])
                      }
                      frame "Property Node" {
                        n929 = Unbundle By Name(w2352) -> ("PropertyNodeMethods"=w2351:T12[])
                      }
                    }
                    n930 = for {
                      tunnel: w2334 -> [w2340] mode=indexing
                      tunnel: [w2342] -> w2335 mode=indexing
                      tunnel: [w2341] -> w2331 mode=indexing
                      tunnel: [w2339] -> w2332 mode=indexing
                      tunnel: [w2338] -> w2330 mode=indexing
                      n931 = Unbundle(w2340) -> ("Name"=w2341:string, "Path"=w2339:path, "DynamicDispatch"=w2338:T14)  [unwired: 3 out]
                      n932 = case shown="\"\"" w2341 {
                        tunnel: [0 -1] -> w2342
                        frame Default {
                        }
                        frame "" {
                        }
                      }
                    }
                    n933 = property on="_Method" class="LstBox (strict)"("Item Names"=w2331, "Item Symbols"=w2335) -> ()  [unwired: 2 in, 2 out]
                  }
                }
              }
              frame True {
                n934 = local write "_AddMessageClass"(FALSE ("_AddMessageClass")) -> ()
                n935 = for {
                  tunnel: w2357 -> [w2361] mode=indexing
                  tunnel: [w2363] -> w2358 mode=indexing
                  tunnel: [w2362] -> w2354 mode=indexing
                  tunnel: [w2360] -> w2355 mode=indexing
                  tunnel: [w2359] -> w2353 mode=indexing
                  n936 = Unbundle(w2361) -> ("Name"=w2362:string, "Path"=w2360:path, "DynamicDispatch"=w2359:T14)  [unwired: 3 out]
                  n937 = case shown="\"\"" w2362 {
                    tunnel: [0 -1] -> w2363
                    frame Default {
                    }
                    frame "" {
                    }
                  }
                }
                n938 = property on="_Method" class="LstBox (strict)"("Item Names"=w2354, "Item Symbols"=w2358) -> ()  [unwired: 2 in, 2 out]
              }
            }
            n939 = Bundle By Name(cluster=w2304, "AF-Method"=w2301, "MethodVIs"=w2298, "MethodItemNames"=w2297, "Methods.DynamicDispatch"=w2296) -> (w2303:T18)
          }
          frame "UpdateIcon:2" {
            w2438 = T29 {"BgIcon"=[], "BgIconOffset"={"X"=0, "Y"=0}, "BgIconMask"=[], "ColorsOkayforiconToBeOnTopOf"=[]}  # BgIcon
            n940 = Unbundle By Name(w2414) -> ("Frame thickness"=w2435:i32, "ConnectorPaneHeight"=w2423:i32[], "BodyIconHeight"=w2424:i32, "MethodIcon"=w2413:u8[][])
            n941 = Unbundle By Name(w2414) -> ("Frame"=w2430:u32, "Frame thickness"=w2421:i32, "HeaderIcon"=w2427:u8[][])
            n942 = local read "_IconSize"() -> (w2431:u16)
            n943 = local read "_BodyBk"() -> (w2417:T1)
            n944 = Unbundle By Name(w2417) -> ("Color"=w2445:u32)
            n945 = Unbundle By Name(w2414) -> ("BgIcon"=w2439:u8[][], "BgIconOffset"=w2440:cluster{"X":i32, "Y":i32}, "BgIconMask"=w2442:u8[], "HeaderBkColor"=w2443:u32)
            n946 = case shown="Default" w2431 {
              tunnel: w2427 -> [w2462 _]
              tunnel: [w2462 _] -> w2428
              frame Default {
              }
              frame 1 {
              }
            }
            n947 = Not Equal?(x=u16 0, y=w2431) -> (x != y?=w2432:bool)
            n948 = Array Size(array=w2428) -> (size(s)=w2425:i32[])
            n949 = Index Array(array=w2425) -> (element=w2426:i32)  [unwired: 1 in]
            n950 = call <resource>:"GDSLvIcon_Convert24bitTo8bitColor.vi"("Color 24bit In"=w2443) -> ("Color out(256)"=w2444:u8)  [unwired: 15 in, 3 out]
            n951 = call <resource>:"GDSLvIcon_Convert24bitTo8bitColor.vi"("Color 24bit In"=w2445) -> ("Color out(256)"=w2446:u8)  [unwired: 15 in, 3 out]
            n952 = Select(t=0, s=w2432, f=0) -> (s? t:f=w2434:i32)
            n953 = Multiply(x=w2435, y=u32 2) -> (x*y=w2436:u32)
            n954 = case shown="1" w2431 {
              selector: w2431 -> [_ w2450 _]
              tunnel: w2424 -> [_ _ _]
              tunnel: w2423 -> [_ w2457 w2460]
              tunnel: [32 ("ImageRows(32)") w2454 w2461] -> w2429
              tunnel: w2426 -> [_ w2453 _]
              tunnel: w2436 -> [_ w2452 w2458]
              frame 0 {
              }
              frame Default {
                n955 = Decrement(x=w2450) -> ()  [unwired: 1 out]
                n956 = Array Subset(array=w2457, length=w2450) -> (w2456:i32[])  [unwired: 1 in]
                n957 = Add Array Elements(numeric array=w2456) -> (sum=w2455:i32)
                n958 = Increment(x=w2452) -> (x+1=w2451:u32)
                n959 = Compound Arithmetic op=ADD(w2451, w2453, w2455) -> (w2454:u32)
              }
              frame 1 {
                n960 = Index Array(array=w2460) -> (element=w2459:i32)  [unwired: 1 in]
                n961 = Compound Arithmetic op=ADD(w2458, w2459) -> (w2461:u32)
              }
            }
            n962 = Build Array(w2444, w2446) -> (w2441:u8[])
            n963 = Bundle By Name(cluster=w2438, "BgIcon"=w2439, "BgIconOffset"=w2440, "BgIconMask"=w2442, "ColorsOkayforiconToBeOnTopOf"=w2441) -> (w2447:T29)
            n964 = call <resource>:"GDSLvIcon_CreateIconPicture.vi"("FrameColor"=w2430, "FrameThickness(1)"=w2421, "HeaderIconIn"=w2428, "BodyIconIn"=w2413, "error in (no error)"=w2419, "ImageRows(32)"=w2429, "BigSizeIcon(x6)"=4, "RowStart(0)"=w2434, "BgIcon"=w2447) -> ("BodyIconOut"=w2410:u8[][], "WholeIconOut"=w2448:u8[][], "LargeIconPictureOut(x6)"=w2437:picture, "error out"=w2418:errorcluster)  [unwired: 5 in, 2 out]
            n965 = local write "_IconPreview"(w2437) -> ()
            n966 = Bundle By Name(cluster=w2414, "CurrentIcon"=w2447, "IconOut"=w2448, "BodyIconOut"=w2410) -> (w2416:T18)
          }
          frame "UpdateIconFromParentMethod" {
            w2495 = T29 {"BgIcon"=[], "BgIconOffset"={"X"=0, "Y"=0}, "BgIconMask"=[], "ColorsOkayforiconToBeOnTopOf"=[]}  # BgIcon
            n967 = Unbundle By Name(w2467) -> ("OverrideMethod"=w2472:path)
            n968 = call <resource>:"GDSLvIcon_AnalyseViIcon.vi"("ViRef/LvCLassRef/LvLibRef/ViPath/2D_Image"=w2472, "error in (no error)"=w2471) -> ("FrameThickness(1)"=w2470:u32, "BodyIcon"=w2469:u8[][], "BodyBkColor"=w2466:u32)  [unwired: 4 in, 11 out]
            n969 = Unbundle By Name(w2467) -> ("Frame"=w2488:u32, "Frame thickness"=w2480:i32, "HeaderIcon"=w2485:u8[][])
            n970 = Unbundle By Name(w2467) -> ("ConnectorPaneHeight"=w2482:i32[])  [unwired: 3 out]
            n971 = local read "_BodyBk"() -> (w2478:T1)
            n972 = Unbundle By Name(w2478) -> ("Color"=w2464:u32)
            n973 = local read "_IconSize"() -> (w2489:u16)
            n974 = call <resource>:"GDSLvIcon_Convert24bitTo8bitColor.vi"("Color 24bit In"=w2464) -> ("Color out(256)"=w2465:u8)  [unwired: 15 in, 3 out]
            n975 = call <resource>:"GDSLvIcon_ReplaceIconColor.vi"("IconIn"=w2469, "OldColor"=w2466, "NewColor"=w2464) -> ("IconOut"=w2468:u8[][])  [unwired: 15 in, 1 out]
            n976 = Unbundle By Name(w2467) -> ("BgIcon"=w2496:u8[][], "BgIconOffset"=w2497:cluster{"X":i32, "Y":i32}, "BgIconMask"=w2499:u8[], "HeaderBkColor"=w2500:u32)
            n977 = case shown="Default" w2489 {
              tunnel: w2485 -> [w2517 _]
              tunnel: [w2517 _] -> w2486
              frame Default {
              }
              frame 1 {
              }
            }
            n978 = Not Equal?(x=u16 0, y=w2489) -> (x != y?=w2490:bool)
            n979 = Array Size(array=w2486) -> (size(s)=w2483:i32[])
            n980 = Index Array(array=w2483) -> (element=w2484:i32)  [unwired: 1 in]
            n981 = call <resource>:"GDSLvIcon_Convert24bitTo8bitColor.vi"("Color 24bit In"=w2500) -> ("Color out(256)"=w2501:u8)  [unwired: 15 in, 3 out]
            n982 = Select(t=0, s=w2490, f=0) -> (s? t:f=w2492:i32)
            n983 = Multiply(x=w2470, y=u32 2) -> (x*y=w2493:u32)
            n984 = case shown="Default" w2489 {
              selector: w2489 -> [_ w2505 _]
              tunnel: w2482 -> [_ w2512 w2515]
              tunnel: [32 ("ImageRows(32)") w2509 w2516] -> w2487
              tunnel: w2484 -> [_ w2508 _]
              tunnel: w2493 -> [_ w2507 w2513]
              frame 0 {
              }
              frame Default {
                n985 = Array Subset(array=w2512, length=w2505) -> (w2511:i32[])  [unwired: 1 in]
                n986 = Add Array Elements(numeric array=w2511) -> (sum=w2510:i32)
                n987 = Increment(x=w2507) -> (x+1=w2506:u32)
                n988 = Compound Arithmetic op=ADD(w2506, w2508, w2510) -> (w2509:u32)
              }
              frame 1 {
                n989 = Index Array(array=w2515) -> (element=w2514:i32)  [unwired: 1 in]
                n990 = Compound Arithmetic op=ADD(w2513, w2514) -> (w2516:u32)
              }
            }
            n991 = Build Array(w2501, w2465) -> (w2498:u8[])
            n992 = Bundle By Name(cluster=w2495, "BgIcon"=w2496, "BgIconOffset"=w2497, "BgIconMask"=w2499, "ColorsOkayforiconToBeOnTopOf"=w2498) -> (w2502:T29)
            n993 = call <resource>:"GDSLvIcon_CreateIconPicture.vi"("FrameColor"=w2488, "FrameThickness(1)"=w2480, "HeaderIconIn"=w2486, "BodyIconIn"=w2468, "error in (no error)"=w2471, "ImageRows(32)"=w2487, "BigSizeIcon(x6)"=4, "RowStart(0)"=w2492, "BgIcon"=w2502) -> ("BodyIconOut"=w2473:u8[][], "WholeIconOut"=w2503:u8[][], "LargeIconPictureOut(x6)"=w2494:picture, "error out"=w2463:errorcluster)  [unwired: 5 in, 2 out]
            n994 = local write "_IconPreview"(w2494) -> ()
            n995 = Bundle By Name(cluster=w2467, "CurrentIcon"=w2502, "IconOut"=w2503, "BodyIconOut"=w2473) -> (w2477:T18)
            n996 = call <vilib>:"Unset Busy.vi"("error in (no error)"=w2463) -> ()  [unwired: 10 in, 1 out]
          }
          frame "Error", "Exit", Default {
            n997 = Unbundle By Name(w2521) -> ("Cancel"=w2520:bool)
            n998 = Unbundle By Name(w2522) -> ("status"=w2519:bool)
            n999 = Or(x=w2520, y=w2519) -> (x .or. y?=w2518:bool)
            n1000 = Bundle By Name(cluster=w2521, "Cancel"=w2518) -> (w2524:T18)
          }
        }
      }
    }
    frame Error {
    }
  }
  "error out" <- w27
  n1001 = call <resource>:"GDSString_AddStatesToQueue.vi"() -> ()  [unwired: 15 in, 1 out]
  n1002 = Generate User Event(user event=w5, event data cluster="Stop" ("Stop")) -> (user event out=w10:refnum<user-event>)  [unwired: 2 in, 1 out]
  n1003 = Destroy User Event(user event=w10) -> ()  [unwired: 1 in, 1 out]
  n1004 = disable-structure shown="Disabled" {
    frame Disabled {
      n1005 = call <resource>:"GDSControl_Enable.vi"() -> ("Enable Property"=w2529:T19)  [unwired: 11 in]
      n1006 = property on="_DynamicDispatch" class="Bool (strict)"("Disabled"=w2529) -> ()  [unwired: 2 in, 2 out]
      n1007 = call <resource>:"GDSControl_Disable.vi"() -> ("Enable Property"=w2530:T19)  [unwired: 11 in]
      n1008 = property on="_DynamicDispatch" class="Bool (strict)"("Disabled"=w2530) -> ()  [unwired: 2 in, 2 out]
    }
    frame Enabled {
    }
  }
  n1009 = stacked-sequence {
    tunnel: w39 -> [w2594]
    tunnel: [w2605] -> w38
    tunnel: [w2574] -> w31
    tunnel: [w2604] -> w32
    tunnel: [w2558] -> w30
    tunnel: [w2578] -> w33
    tunnel: [w2602] -> w34
    tunnel: [w2601] -> w35
    tunnel: [w2542] -> w29
    tunnel: [w2531] -> w28
    tunnel: [w2596] -> w26
    tunnel: [w2597] -> w25
    tunnel: [w2532] -> w22
    tunnel: [w2533] -> w21
    tunnel: [w2567] -> w20
    tunnel: [w2566] -> w19
    tunnel: [w2546] -> w14
    frame #0 {
      n1010 = Unbundle By Name(w2594) -> ("OverrideMethodsIdx"=w2534:i32[], "AF-Method"=w2561:i32, "AllOverrideMethods"=w2560:path[], "AF"=w2565:bool, "ActorVersion"=w2564:string, "IsAPropertyDefinitionVI"=w2552:bool[])
      n1011 = Unbundle By Name(w2594) -> ("Signatures.SignatureName"=w2590:string[], "Signatures.SignatureText"=w2591:string[], "Signatures.Current"=w2593:i32)
      n1012 = Unbundle By Name(w2594) -> ("FolderNames"=w2600:string[], "IconDetails"=w2567:T5, "Open"=w2597:bool, "Cancel"=w2605:bool, "RelFolderPath"=w2557:path[], "BodyIconOut"=w2601:u8[][], "MethodNames"=w2555:string[])
      n1013 = local read "_MethodSignature"() -> (w2589:u16)
      n1014 = local read "_Visibility"() -> (w2603:T7)
      n1015 = local read "_MethodName"() -> (w2536:string)
      n1016 = local read "_MethodType"() -> (w2598:T2)
      n1017 = property on="_Visibility" class="RadioBtnsControl (strict)"() -> ("Disabled"=w2562:T19)  [unwired: 2 in, 2 out]
      n1018 = local read "_MethodType"() -> (w2550:T2)
      n1019 = local read "_MethodLocation"() -> (w2599:i32)
      n1020 = Index Array(array=w2600, index=w2599) -> (element=w2556:string)
      n1021 = Match Pattern(string=w2536, regular expression="\\2E[Vv][Ii][Mm]*") -> (before substring=w2535:string)  [unwired: 1 in, 3 out]
      n1022 = local read "_Method"() -> (w2554:i32[])
      n1023 = Array Size(array=w2554) -> (size(s)=w2553:i32)
      n1024 = case shown="-1" w2561 {
        selector: w2561 -> [w2619 _]
        tunnel: w2598 -> [_ w2630]
        tunnel: w2560 -> [_ w2629]
        tunnel: [_ w2628] -> w2595
        tunnel: w2594 -> [w2621 w2627]
        tunnel: [w2617 w2626] -> w2588
        tunnel: w2535 -> [_ w2625]
        tunnel: w2553 -> [_ w2624]
        tunnel: w2552 -> [_ w2623]
        tunnel: [_ w2622] -> w2548
        frame 0, Default {
          n1025 = Unbundle By Name(w2621) -> ("AF-Methods"=w2620:cluster{T12[]}[])
          n1026 = Index Array(array=w2620, index=w2619) -> (element=w2618:cluster{T12[]})
          n1027 = Unbundle(w2618) -> (w2617:T12[])
        }
        frame -1 {
          n1028 = case shown="\"Normal Method\", Default" w2630 {
            tunnel: w2629 -> [_ w2641 _ _]
            tunnel: [_ w2640 w2651 w2672] -> w2628
            tunnel: w2627 -> [w2632 w2639 w2650 w2671]
            tunnel: [w2631 w2638 w2649 w2670] -> w2626
            tunnel: w2625 -> [_ _ _ w2663]
            tunnel: w2624 -> [_ _ w2644 w2660]
            tunnel: w2623 -> [_ w2637 _ _]
            tunnel: [_ w2636 _ _] -> w2622
            frame "Normal Method", Default {
              n1029 = Unbundle By Name(w2632) -> ("NormalMethods"=w2631:T12[])
            }
            frame "Override Method" {
              n1030 = local read "_OverrideMethods"() -> (w2635:i32)
              n1031 = Unbundle By Name(w2639) -> ("OverrideMethods"=w2638:T12[], "OverrideMethodsIdx"=w2634:i32[])
              n1032 = Index Array(array=w2634, index=w2635) -> (element=w2633:i32)
              n1033 = Index Array(array=w2637, index=w2633) -> (element=w2636:bool)
              n1034 = Index Array(array=w2641, index=w2633) -> (element=w2640:path)
            }
            frame "Property Method" {
              n1035 = local read "_Property"() -> (w2643:string[])
              n1036 = Unbundle By Name(w2650) -> ("PropertyMethods"=w2649:T12[])
              n1037 = for {
                tunnel: w2643 -> [w2656] mode=indexing
                tunnel: w2644 -> [w2655]
                shift-right: [w2654] -> w2642
                shift-left: string[] [] -> [w2653]
                n1038 = Initialize Array(w2656, w2655) -> (w2652:string[])
                n1039 = Build Array (concatenate)(w2653, w2652) -> (w2654:string[])
              }
              n1040 = Bundle(cluster=T9 {"AttributeNames"=[], "PropertyNode"=FALSE, "FolderNames"=[]}, "AttributeNames"=w2642, "PropertyNode"=FALSE) -> (w2647:T9)  [unwired: 1 in]
              n1041 = To Variant(anything=w2647) -> (Variant=w2651:variant)
            }
            frame "Property Node" {
              w2659 = string[] []
              n1042 = Unbundle By Name(w2671) -> ("PropertyNodeMethods"=w2670:T12[])
              n1043 = local read "_Property"() -> (w2658:string[])
              n1044 = Spreadsheet String To Array(delimiter (Tab)="/", format string="%s", spreadsheet string=w2663, array type (2D Dbl)=string[] []) -> (array=w2664:string[])
              n1045 = for {
                tunnel: w2658 -> [w2677] mode=indexing
                tunnel: w2660 -> [w2676]
                shift-right: [w2675] -> w2657
                shift-left: w2659 -> [w2674]
                n1046 = Initialize Array(w2677, w2676) -> (w2673:string[])
                n1047 = Build Array (concatenate)(w2674, w2673) -> (w2675:string[])
              }
              n1048 = for {
                tunnel: w2664 -> [w2682] mode=indexing
                tunnel: w2660 -> [w2681]
                shift-right: [w2680] -> w2661
                shift-left: w2659 -> [w2679]
                n1049 = Initialize Array(w2682, w2681) -> (w2678:string[])
                n1050 = Build Array (concatenate)(w2679, w2678) -> (w2680:string[])
              }
              n1051 = Bundle(cluster=T9 {"AttributeNames"=[], "PropertyNode"=FALSE, "FolderNames"=[]}, "AttributeNames"=w2657, "PropertyNode"=TRUE, "FolderNames"=w2661) -> (w2668:T9)
              n1052 = To Variant(anything=w2668) -> (Variant=w2672:variant)
            }
          }
        }
      }
      n1053 = case shown="\"Disabled and Grayed Out\"" w2562 {
        tunnel: w2603 -> [_ w2735]
        tunnel: [GOOP300_MethodScopeType."Use Parent Folder Scope" ("Scope/Visibility") w2734] -> w2602
        frame "Disabled and Grayed Out" {
        }
        frame Default {
          n1054 = case shown="\"Community\"" w2735 {
            tunnel: [GOOP300_MethodScopeType."Protected" ("Scope/Visibility") GOOP300_MethodScopeType."Private" ("Scope/Visibility") GOOP300_MethodScopeType."Public" ("Scope/Visibility") GOOP300_MethodScopeType."Community" ("Scope/Visibility")] -> w2734
            frame "Protected" {
            }
            frame "Private" {
            }
            frame "Public" {
            }
            frame "Community" {
            }
          }
        }
      }
      n1055 = Index Array(array=w2557, index=w2599) -> (element=w2559:path)
      n1056 = Not Equal?(x=w2593, y=w2589) -> (x != y?=w2592:bool)
      n1057 = local read "_MethodDescription"() -> (w2604:string)
      n1058 = Equal?(x=T2."Property Node" ("_MethodType"), y=w2550) -> (x = y?=w2549:bool)
      n1059 = Build Array(w2535) -> (w2580:string[])
      n1060 = Empty Array?(array=w2555) -> (empty?=w2579:bool)
      n1061 = Select(t=w2580, s=w2579, f=w2555) -> (s? t:f=w2540:string[])
      n1062 = local read "_DynamicDispatch"() -> (w2531:bool)
      n1063 = local read "_MustCallParent"() -> (w2533:bool)
      n1064 = local read "_MustOverride"() -> (w2532:bool)
      n1065 = Or(x=w2549, y=w2548) -> (x .or. y?=w2547:bool)
      n1066 = case shown="True" w2547 {
        tunnel: w2559 -> [_ w2616]
        tunnel: [w2613 w2616] -> w2558
        tunnel: w2557 -> [w2614 _]
        tunnel: w2556 -> [_ w2615]
        tunnel: [w2612 w2615] -> w2541
        frame True {
          w2612 = "properties"
          n1067 = Index Array(array=w2614) -> ()  [unwired: 1 in, 1 out]
          n1068 = String To Path(string=w2612) -> (path=w2613:path)
        }
        frame False {
        }
      }
      n1069 = local read ".vim"() -> (w2538:bool)
      n1070 = case shown="True" w2538 {
        tunnel: w2540 -> [w2606 w2608]
        tunnel: [w2606 w2607] -> w2539
        frame False {
        }
        frame True {
          n1071 = for {
            tunnel: w2608 -> [w2611] mode=indexing
            tunnel: [w2609] -> w2607 mode=indexing
            n1072 = Concatenate Strings(w2611, ".vim" ("string")) -> (w2609:string)
          }
        }
      }
      n1073 = for {
        tunnel: w2588 -> [w2699]
        tunnel: [w2697] -> w2587
        tunnel: [w2696] -> w2571 mode=indexing
        tunnel: [w2695] -> w2586
        tunnel: [w2694] -> w2546
        tunnel: [w2693] -> w2585
        tunnel: [w2692] -> w2584
        tunnel: w2554 -> [w2691] mode=indexing
        n1074 = Index Array(array=w2699, index=w2691) -> (element=w2698:T12)
        n1075 = Unbundle By Name(w2698) -> ("Type"=w2697:T13, "Name"=w2695:string, "Path"=w2694:path, "ExtraName"=w2692:string, "Data"=w2693:variant)
        n1076 = Strip Path(path=w2694) -> (name=w2696:string)  [unwired: 1 out]
      }
      n1077 = case shown="True" w2592 {
        tunnel: w2591 -> [_ w2724]
        tunnel: w2590 -> [_ w2723]
        tunnel: w2589 -> [_ w2722]
        frame False {
        }
        frame True {
          n1078 = Array Size(array=w2724) -> (size(s)=w2730:i32)
          n1079 = call <resource>:"GOOP_GetGDSConfigFolder.vi"() -> ("GDSFolderPath"=w2731:path)
          n1080 = Max & Min(x=w2730, y=w2722) -> (min(x,y)=w2729:i32)  [unwired: 1 out]
          n1081 = Build Path(base path=w2731, name or relative path="MethodSignatures.xml") -> (appended path=w2727:path)
          n1082 = Bundle("SignatureName"=w2723, "SignatureText"=w2724, w2729) -> (w2728:T48)  [unwired: 1 in]
          n1083 = Delete(path (use dialog)=w2727) -> (deleted path=w2726:path)  [unwired: 4 in, 2 out]
          n1084 = Flatten To XML(6:w2728) -> (2:w2725:string)
          n1085 = Write to Text File(file (use dialog)=w2726, text=w2725) -> ()  [unwired: 2 in, 3 out]
        }
      }
      n1086 = case shown="True" w2565 {
        tunnel: [_ w2687] -> w2566
        tunnel: w2564 -> [_ w2685]
        tunnel: cluster{"Add":bool, "ActorVersion":string} {"Add"=FALSE, "ActorVersion"=""} ("cluster") -> [_ w2683]
        frame False {
        }
        frame True {
          n1087 = Bundle(cluster=w2683, "Add"="_AddMessageClass", "ActorVersion"=w2685) -> (w2684:cluster{"Add":bool, "ActorVersion":string})
          n1088 = To Variant(anything=w2684) -> (Variant=w2687:variant)
        }
      }
      n1089 = Array Size(array=w2540) -> (size(s)=w2569:i32)
      n1090 = Array Size(array=w2571) -> (size(s)=w2570:i32)
      n1091 = Equal?(x=w2541, y="<class root>") -> (x = y?=w2544:bool)
      n1092 = Divide(x=w2569, y=w2570) -> (x/y=w2568:dbl)
      n1093 = for {
        N: w2568 -> [_]
        shift-right: [w2689] -> w2573
        shift-left: string[] [] -> [w2690]
        tunnel: w2571 -> [w2688]
        n1094 = Build Array (concatenate)(w2690, w2688) -> (w2689:string[])
      }
      n1095 = Select(t="", s=w2544, f=w2541) -> (s? t:f=w2542:string)
      n1096 = case shown="\"DesignPattern\"" w2587 {
        selector: w2587 -> [_ w2708 _ _]
        tunnel: [w2700 w2706 w2713 w2721] -> w2596
        tunnel: w2595 -> [w2700 _ _ _]
        tunnel: w2586 -> [_ _ w2712 w2719]
        tunnel: w2546 -> [_ w2707 _ w2718]
        tunnel: w2585 -> [_ _ w2711 w2717]
        tunnel: w2584 -> [_ _ _ w2715]
        tunnel: w2560 -> [_ w2705 _ _]
        tunnel: w2534 -> [_ w2703 _ _]
        frame "Normal", Default {
        }
        frame "AF-Method" {
          n1097 = local read "_OverrideMethods"() -> (w2702:i32)
          n1098 = Index Array(array=w2703, index=w2702) -> (element=w2701:i32)
          n1099 = Index Array(array=w2705, index=w2701) -> (element=w2704:path)
          n1100 = Bundle("Type"=w2708, "Path"=w2707, "Path"=w2704) -> (w2706:cluster{"Type":T13, "Path":path, "Path":path})  [unwired: 1 in]
        }
        frame "MethodPlugIn" {
          n1101 = Variant To Data(type=" ", Variant=w2711) -> (data=w2709:string)  [unwired: 1 in, 1 out]
          n1102 = Bundle(cluster=T47 {"PlugInName"="", "MethodSelected"=""}, "PlugInName"=w2709, "MethodSelected"=w2712) -> (w2713:T47)
        }
        frame "DesignPattern" {
          n1103 = Bundle(cluster=T10 {"Type"=enum."DesignPattern", "ID"="", "Version"="", "Path"=path "", "Name"="", "Data"=variant}, "Type"=GDSLvClass_PlugInTypes."DesignPattern", "ID"=w2719, "Path"=w2718, "Name"=w2715, "Data"=w2717) -> (w2721:T10)  [unwired: 1 in]
        }
      }
      n1104 = Array To Spreadsheet String(delimiter (Tab)="\n", array=w2539, 3:"%s" ("format string")) -> (spreadsheet string=w2576:string)
      n1105 = call <vilib>:"Trim Whitespace.vi"("string"=w2576) -> ("trimmed string"=w2574:string)  [unwired: 1 in]
      n1106 = Array To Spreadsheet String(delimiter (Tab)="\n", array=w2573, 3:"%s" ("format string")) -> (spreadsheet string=w2582:string)
      n1107 = call <vilib>:"Trim Whitespace.vi"("string"=w2582) -> ("trimmed string"=w2578:string)  [unwired: 1 in]
    }
  }
  "Cancelled" <- w38
  n1108 = Bundle By Name(cluster=T3 {"MethodName"="", "RelativeMethodPath"=path "", "MethodDescription"="", "Scope/Visibility"=enum."Use Parent Folder Scope", "MethodTemplateName"="", "IconOut"=[], "RelativeProjectClassPath"="", "OpenViAfterCreation"=FALSE, "DynamicDispatchVi"=FALSE, "ExtraCreateParameters"=variant, "MustOverride"=FALSE, "MustCallParent"=FALSE, "IconDetails"={"IconSize"=enum."Full", "ImageRows(32)"=0, "ConnectorPaneHeight"=[]}, "AF-Option"=variant, "TemplatePath"=path ""} ("CreateMethodData"), "IconDetails"=w20, "RelativeProjectClassPath"=w29, "OpenViAfterCreation"=w25, "RelativeMethodPath"=w30, "MethodName"=w31, "MethodDescription"=w32, "IconOut"=w35, "Scope/Visibility"=w34, "MethodTemplateName"=w33, "DynamicDispatchVi"=w28, "ExtraCreateParameters"=w26, "MustOverride"=w22, "MustCallParent"=w21, "AF-Option"=w19, "TemplatePath"=w14) -> (→"CreateMethodData":T3)
  "ClassWriterNative" <- "ClassWriterNative"
  "ClassItemRefOut" <- "ClassItemRefIn"
  "_DubMethodName" <- "" ("_DubMethodName")
  "_MethodsLocationOverrideInfo" <- "" ("_MethodsLlocationOverrideInfo")
